vi "Process.vi"(8 "error in":errorcluster, 11 "Lockin.UI":refnum<class "Instrument UI.Lockin.lvclass">) -> (0 "error out":errorcluster, 3 "Lockin.UI out":refnum<class "Instrument UI.Lockin.lvclass">)   [LabVIEW 2019, in "Instrument.Lockin.lvlib" / "Instrument UI.Lockin.lvclass"]
doc: "---------------------------------------------------------------\nJKI State Machine Objects™\nhttp://jki.net/state-machine-objects/\nCopyright (C) 2005-2015, JKI <info@jki.net>\nALL RIGHTS RESERVEDJKI State Machine Objects (SMO) 1.0.0.5\nJKI - JKI\nCopyright (c) 2016, JKI"
uses:
  Instrument UI.Lockin.lvclass
  Instrument.DAQ/Typedefs/DAQ.Calibration--Cluster--Array.ctl
  Instrument.DAQ/Typedefs/DAQ.Calibration--Cluster.ctl
  Instrument.Lockin/Typedefs/Results Type--Enum.ctl
  Instrument.DAQ/Typedefs/Channel.Gain--Cluster--Array.ctl
  Instrument.DAQ/Typedefs/Channel.Gain--Cluster.ctl
  Instrument.DAQ/Typedefs/Sweep.Channel--Cluster--Array.ctl
  Instrument.DAQ/Typedefs/Sweep.Channel--Cluster.ctl
  Instrument.DAQ/Typedefs/Sweep.Pattern--Enum.ctl
  Instrument.DAQ/Typedefs/DAQ.Configuration--Cluster--Array.ctl
  Instrument.DAQ/Typedefs/DAQ.Configuration--Cluster.ctl
  Instrument.DAQ/Typedefs/DAQ.Config.AO.Range--enum.ctl
  Instrument.DAQ/Typedefs/DAQ.TerminalConfiguration--ring.ctl
  Instrument.DAQ/Typedefs/DAQ.Config.AI.Range--enum.ctl
  Instrument.DAQ/Typedefs/DAQ.Config.AI.Coupling--enum.ctl
  Instrument.DAQ/Typedefs/DAQ.Sampling.Fs Mode--enum.ctl
  Instrument.DAQ/Typedefs/Simulation Mode--enum.ctl
  Instrument.DAQ/Typedefs/AI.Channel--Cluster--Array.ctl
  Instrument.DAQ/Typedefs/AI.Channel--Cluster.ctl
  Instrument.DAQ/Typedefs/AO.Channel--Cluster--Array.ctl
  Instrument.DAQ/Typedefs/AO.Channel--Cluster.ctl
  Instrument.DAQ/Typedefs/AO.Channel.Function--Enum.ctl
  Instrument.DAQ/Typedefs/REF.Channel--Cluster--Array.ctl
  Instrument.DAQ/Typedefs/REF.Channel--Cluster.ctl
  Typedefs/Display-Enum.ctl
  C:/Program Files/National Instruments/LabVIEW 2019/vi.lib/JKI/JKI SMO/SMO/SMO.lvclass
  C:/Program Files/National Instruments/LabVIEW 2019/user.lib/LevyLab/Instrument Framework/Instrument UI/Instrument UI.lvclass
  C:/Program Files/National Instruments/LabVIEW 2019/vi.lib/JKI/JKI SMO/SMO.UI/SMO.UI.lvclass
  Instrument.DAQ/Typedefs/DAQ.Sampling.Sample Mode--Ring.ctl
  Instrument.DAQ/Typedefs/State--enum.ctl
  Instrument.Lockin/Typedefs/API/Lockin.setSweep_Table--cluster.ctl
  Instrument.Lockin/Typedefs/Offset Mode--Enum.ctl
  Instrument.DAQ/Typedefs/PrivateEvents--DAQ.setCalibration.ctl
  Instrument.DAQ/Typedefs/Status--enum.ctl
  <userlib>/LevyLab/Instrument Framework/Instrument UI/Instrument UI.lvclass/Instrument UI.ctl
  Instrument.Lockin/Instrument.Lockin.lvclass
  C:/Program Files/National Instruments/LabVIEW 2019/user.lib/LevyLab/Instrument Framework/Instrument/Instrument.lvclass
  Typedefs/UI.Configuration--Cluster.ctl
  Instrument.DAQ/Typedefs/Configuration.Channels--Cluster.ctl
  Instrument.DAQ/Typedefs/DAQ.Sampling--Cluster.ctl
  Instrument.DAQ/Typedefs/DAQ.Sampling.Sampling--Cluster.ctl
  Instrument.DAQ/Typedefs/Configuration.Prefilter--Cluster.ctl
  Instrument.DAQ/Typedefs/Channel.GainsAndOffsets--Cluster.ctl
  Instrument.DAQ/Typedefs/Configuration.AmplitudeLimit--Cluster.ctl
  Instrument.DAQ/Typedefs/Configuration.DCLimit--Cluster.ctl
  Instrument.DAQ/Typedefs/Configuration.LinkFrequencies--Cluster.ctl
  Instrument.DAQ/Typedefs/Sweep.Configuration--Cluster.ctl
  Instrument.DAQ/Typedefs/Configuration.DutyCycle--Cluster.ctl
  Instrument.Lockin/Typedefs/Lockin.getAllData--Cluster.ctl
  Instrument.DAQ/Typedefs/PublicEvents--DAQ.getWaveforms.ctl
  Instrument.DAQ/Typedefs/Results--Cluster.ctl
  Instrument.DAQ/Typedefs/PublicEvents--DAQ.getSweepWaveforms.ctl
  <userlib>/LevyLab/Configuration/Configuration.lvclass
  Typedefs/UI.References--Cluster.ctl
  Typedefs/UI.References.Booleans--Cluster.ctl
  Typedefs/UI.References.Clusters--Cluster.ctl
  Typedefs/UI.References.Graphs--Cluster.ctl
  <userlib>/LevyLab/Configuration/Configuration.lvclass/Configuration.ctl
  <vilib>/JKI/JKI SMO/SMO/SMO.lvclass/SMO.ctl
  <vilib>/JKI/JKI SMO/SMO.UI/SMO.UI.lvclass/SMO.UI.ctl
  Instrument.Lockin/Typedefs/API/Lockin.setState--cluster.ctl
  Instrument.Lockin/Typedefs/API/Lockin.Commands--Enum.ctl
  Instrument.Lockin/Typedefs/API/Lockin.Commands.Local--Enum.ctl
  Instrument.DAQ/Typedefs/PrivateEvents--DAQ.showUI.ctl
  Instrument.Lockin/Typedefs/API/Lockin.setLogMode--cluster.ctl
  Instrument.Lockin/Typedefs/API/Lockin.setSamplingMode--cluster.ctl
  Instrument.Lockin/Typedefs/API/Lockin.setSamplingFsMode--cluster.ctl
  ea889f97-4432-4e18-8daa-f8276c71e6b3.vi
  e313e854-8cc0-44b2-b8a5-b0d9dd449797.vi
  f60e4b8a-05f4-439c-aeb3-da82266228cf.vi
  5a499ed1-b987-4b60-a17a-49cbc4aa87e6.vi
  11ce9ad4-6d29-4ca4-b8bb-b11228104e6f.vi
  a8738246-2ac0-499e-83b1-af72f8904bf5.vi
  <vilib>/JKI/JKI SMO/SMO/Private/ReftoDVR--SMO.vi
  <vilib>/JKI/JKI SMO/SMO.UI/SMO.UI.ReftoDVR.vi
  11ce9ad4-6d29-4ca4-b8bb-b11228104e6f.vi/189031a7-82a1-4f0a-9ed5-d68f3439fd4c.vi
  11ce9ad4-6d29-4ca4-b8bb-b11228104e6f.vi/de7eedf1-e1e8-4423-8aaa-e1093bc59ae0.vi
  <vilib>/Platform/browser.llb/Open URL in Default Browser (string).vi
  private/Set Plot Visibility (WDTWFGraph).vi
  <vilib>/measure/matone.llb/Extract Single Tone Information 1 Chan.vi
  private/Set Plot Color (WFChart2D).vi
  private/Set Legend (WDTWFGraph).vi
  <vilib>/Waveform/WDTOps.llb/WDT Waveform Duration DBL.vi
  <vilib>/Utility/Data Type/Get Type Information.vi
  <vilib>/Utility/Data Type/Get Numeric Information.vi
  <userlib>/_OpenG.lib/lvdata/lvdata.llb/Unwrap VVariant__ogtk.vi
  <vilib>/JDP Science/JSONtext/Variant to JSON Text.vi
  <userlib>/LevyLab/Instrument Framework/Instrument/API/Instrument.sendMessageToProcess (string).vi
  <userlib>/LevyLab/Instrument Framework/Instrument/Instrument.lvclass
  <vilib>/JDP Science/JSONtext/LVClass Serializer/JSONtext LVClass Serializer.lvclass
  <userlib>/LevyLab/Instrument Framework/Instrument UI/Instrument UI.lvclass
  Instrument.DAQ/Instrument.DAQ.lvclass
  <vilib>/measure/NI_MAPro.lvlib
  <vilib>/JKI/JKI SMO/SMO/SMO.lvclass
  <vilib>/JKI/JKI SMO/SMO.UI/SMO.UI.lvclass
  Lockin.Utilities/Lockin.Utilities.lvlib
  C:/Program Files/National Instruments/LabVIEW 2019/user.lib/LevyLab/Instrument Framework/Instrument Types/Lockin/Instrument.LockinAPI.lvclass
  private/Set All Plot Visibility (WFGraph).vi
  private/Set All Plot Visibility (XYGraph).vi
  private/Get Plot Visibility (WFGraph).vi
  private/Set Plot Visibility (WFGraph).vi
  private/Set Plot Visibility (XYGraph).vi
  private/Set Legend (WFGraph).vi
  private/Set Plot Color (WDTWFGraph).vi
  private/Set Plot Color (WFGraph).vi
  private/Set Legend (XYGraph).vi
  private/Set Plot Color (XYGraph).vi
  <vilib>/measure/maspectr.llb/FFT Power Spectrum and PSD for N Chan.vi
panel:
  out "Version":string="vDevelopment" caption="V"
  in  "Fs Multiplier":dbl=5000.0 format="%#_13g"
  in  "Refresh Rate (Hz)":dbl=10.0 format="%#_13g"
  in  "Decimate":enum16{"1", "10", "100", "1000"}(ring) caption="Enum 3"
  in  "Decimation (pre DSP)":i32=1
  in  "Decimation (post DSP)":i32=1
  in  "....................State....................":bool
  in  "....................Graph and UI....................":bool
  in  "....................DAQ and Channel....................":bool
  in  "....................Dynamic Events....................":bool
  in  "Left Tab":T1(tab)=enum."DAQ Settings"
  out "-3dB BW (Hz)":dbl=50.0
  out "Noise BW (Hz)":dbl=50.0
  out "Settling Time (s)":dbl=50.0
  in  "REF Channels":T2 {"Roll-Off" min=1 max=4; "TC" min=1e-06 max=100.0 format="%#_3p"; "Phase" format="%#_3p"; "Frequency" min=1e-06 max=102400.0 format="%#_6p"; "Channel" min=1}
  in  "f link (Hz)":dbl=13.0 format="%#_6p"
  in  "Link f?":bool
  in  "Limit DC?":bool
  in  "AO DC Limit":dbl=0.009999999 caption="DC limit" format="%#_6p"
  in  "Limit AC?":bool
  in  "AC Limit":dbl=0.009999999 caption="AC limit" format="%#_6p"
  in  "duty cycle (%)":dbl=50.0
  in  "Disable All":bool
  in  "Enable All":bool
  in  "AI Channels":T4 {"reference index" min=1; "References" items=["", "1", "2", "3", "4", "5", "6", "7", "8", "9"]; "Channel" min=1}
  in  "AO Channels":T6 {"Phase" format="%#_3g"; "Frequency" min=0.0001 max=200000.0 format="%#_6p"; "Offset" format="%#_6p"; "Amplitude" min=0.0 max=10.0 format="%#_6p"}
  in  "Measure Offset":bool caption="Measure"
  in  "Remove Offset":bool caption="Remove"
  out "Fs Output (S/s)":dbl=100.0
  in  "Fs (S/s) (buffer)":dbl=204800.0 format="%#_13g"
  in  "#s (S) (buffer)":i32=20480
  in  "Show DAQ UI":bool
  out "Fs (S/s)":dbl=10.0 format="%#_13g"
  out "#s (S)":i32=10
  in  "DAQ Config":T9 {"AI terminal config" items=[""=-1, "differential"=10106, "pseudodifferential"=12529]; "AI.Coupling" items=[""=0, "AC"=10045, "DC"=10050, "GND"=10066]; "AO terminal config" items=[""=-1, "differential"=10106, "pseudodifferential"=12529]}
  in  "Auto DAQ":bool caption="Auto Configure"
  in  "Fs Mode":T15
  in  "Logging":bool
  in  "AI Simulation mode":T16=enum."AI = noise*AO"
  in  "Reset Phase":bool
  in  "LP f (Hz)":dbl=100.0 format="%.3p"
  in  "Line":bool
  in  "Lowpass":bool
  in  "PLL AI Channel":i32=1 caption="AI Channel"
  in  "Enable PLL":bool caption="Enable"
  in  "Input Gain":T17
  in  "Output Gain":T17
  in  "Input Offsets":T17 {"Gain" format="%#_3p"}
  in  "Route Signal Type":T19 caption="Signal Type"
  in  "Route Ref Channel":i32=1 caption="Ref Channel"
  in  "Route AI Channel":i32=1 caption="AI Channel"
  out "Route Output (V)":dbl caption="Output (V)"
  in  "Route AO Channel":i32=1 caption="AO Channel" min=1
  in  "Enable Route":bool caption="Enable"
  in  "Sweep Pattern":cluster{"Channel":u16, "Sweep Pattern":dbl[]}[](array[cluster])=[{"Channel"=0, "Sweep Pattern"=[]}] {"Sweep Pattern" format="%#_3p"; "Channel" min=1 max=128}
  in  "Sweep Channels":T20=[{"Enable?"=FALSE, "Channel"=0, "Start"=0.0, "End"=0.1, "Pattern"=enum."Table", "Table"=[]}] {"Table" format="%#_1f"; "Channel" min=1 max=128; "Start" format="%#_6p"; "End" format="%#_6p"}
  in  "Sweep Time (s)":dbl=20.0
  in  "Initial Wait (s)":dbl=1.0
  out "Sweep Timer (s)":dbl caption="Timer (s)"
  in  "Return to Start?":bool
  out "System Serial Number":string caption="SMO State"
  out "Application Version":string caption="SMO State"
  out "Status":string
  out "Sampling Status":u32(colorbox)
  out "State Queue":string
  out "Sampling Status":string="Good"
  out "State History":string
  out "Wfm Refresh Time (ms)":u32=103
  out "Inst.DAQ State":string caption="SMO State"
  out "UI Refresh Time (ms)":u32=103
  out "Sweep Time":dbl format="%<%I:%M:%S %p %m/%d/%Y>T"
  out "State Time":dbl format="%<%I:%M:%S %p %m/%d/%Y>T"
  out "Cal Info":T23 {"DevTemp" format="%.1f"; "SelfCal.LastTemp" format="%.1f"; "SelfCal.LastDate/Time" format="%<%I:%M %p %m/%d/%Y>T"}
  in  "Get Calibration":bool
  in  "Self Calibrate":bool
  in  "Tab Control 3":enum32{"Page 1"}(tab)
  out "mean (V)":dbl format="%_3p"
  out "X (V)":dbl format="%_3p"
  out "Y (V)":dbl format="%_3p"
  in  "channel-reference":u16(ring) items=["AI1 REF 1"]
  out "R (V)":dbl format="%_3p"
  out "theta (°)":dbl format="%_3p"
  in  "Close":bool
  out "String":string
  in  "Pause":bool
  in  "Reset":bool
  in  "Start":bool
  in  "Help":bool
  in  "Start Sweep":bool
  in  "Stop Sweep":bool
  in  "Right Tab":T25(tab)
  in  "Sync?":bool
  in  "Sync Ch":i32=1
  out "f (Hz)":string
  out "phi (°)":string
  in  "Output":enum16{"AO", "REF"}(ring) caption="Enum 3"
  in  "Input":enum16{"Device", "ADC"}(ring) caption="Enum 3"
  out "REF Graph":waveform(dbl)[](graph)
  in  "AO Graph All":bool
  in  "AO Graph None":bool
  in  "AI Graph All":bool
  in  "AI Graph None":bool
  out "AI Graph":waveform(dbl)[](graph)
  in  "X Scale":enum16{"time", "samples"}(ring) caption="Enum 3"
  out "AO Graph":waveform(dbl)[](graph)
  in  "REF Graph None":bool
  in  "REF Graph All":bool
  out "Lockin 1":waveform(dbl)[](graph)
  in  "Display 2":T26 caption="Enum 3"
  in  "Y/Theta Range":dbl caption="Range" format="%#_6p"
  in  "Display 1":T26 caption="Enum 3"
  in  "X/R Range":dbl caption="Range" format="%#_6p"
  out "Lockin 2":waveform(dbl)[](graph)
  in  "Lockin Graph All":bool
  in  "Lockin Graph None":bool
  out "Results":string[][](table)
  out "Lockin XY":cluster{dbl[], dbl[]}[](graph)
  in  "XY Range":dbl caption="Range" format="%#_6p"
  in  "Lockin Graph None 2":bool
  in  "Lockin Graph All 2":bool
  out "Sweep AI":waveform(dbl)[](graph)
  out "Sweep AO":waveform(dbl)[](graph)
  out "Sweep Y":waveform(dbl)[](graph)
  out "Sweep X":waveform(dbl)[](graph)
  in  "chart?":bool=TRUE
  in  "chart all?":bool=TRUE
  in  "PS Display":enum16{"AO", "AI", "X", "Y", "R", "Theta"}(ring) caption="Enum 3"
  in  "# averages":u32=10 min=1
  in  "weighting mode":enum16{"Linear", "Exponential"}(ring)=enum."Exponential"
  in  "averaging mode":T27(ring)=enum."RMS averaging"
  in  "window":u32(ring)=1 items=["Rectangle"=0, "Hanning"=1, "Hamming"=2, "Blackman-Harris"=3, "Exact Blackman"=4, "Blackman"=5, "Flat Top"=6, "4 Term B-Harris "=7, "7 Term B-Harris"=8, "Low Sidelobe"=9, "Blackman Nuttall"=11, "Triangle"=30, "Bartlett-Hanning"=31, "Bohman"=32, "Parzen"=33, "Welch"=34, "Kaiser"=60, "Dolph-Chebyshev"=61, "Gaussian"=62]
  in  "export mode":u16(ring)=1 items=["Power Spectrum", "Power Spectral Density"]
  in  "restart":bool
  out "done?":bool=TRUE
  out "PS Waveform":cluster{"f0":dbl, "df":dbl, "magnitude":dbl[]}[](graph)
  out "averages":dbl=180.0
  out "PS Chart":dbl[][](graph)
  # "Lockin UI"
  # "For instructions on how to use the JKI State Machine Objects, examples and video tutorials, visit:\nhttp://jki.net/state-machine-objects/\n\nJKI State Machine Objects™\nhttp://jki.net/state-machine-objects/\nCopyright (C) 2005-2015, JKI <info@jki.net>\nALL RIGHTS RESERVED"
  # "- Choose an input lockin channel and value (X,Y, etc) and it will be written as a DC value to an output channel of your choosing.\n- Output is scaled by the input amplifier gain."
  # "Output"
  # "Input"
  # ">> DEVICE >>"
  # "(*)"
  # "ch"
  # "AC (V)"
  # "DC (V)"
  # "f (Hz)"
  # "phase (°)"
  # "function"
  # "sweep"
  # "(*)"
  # "ch"
  # "1     2    3"
  # "References"
  # "Offset"
  # "Output Settings"
  # "Reference"
  # "Reference Filter"
  # "ch"
  # "f (Hz)"
  # "phase (°)"
  # "TC (s)"
  # "order (n)"
  # "DAQ Channels"
  # "Device"
  # "AO"
  # "AI"
  # "terminals"
  # "ch"
  # "ch"
  # "range"
  # "range"
  # "coupling"
  # "terminals"
  # "Sampling"
  # "Pre-Filters"
  # "Simulation"
  # "Push \"Reset Acquisiton\" below when you want to apply new settings"
  # "not used during process-ing"
  # "DAQ"
  # "Logging"
  # "Output Gain"
  # "Input Offset / Gain"
  # "Route Lockin Input to Output"
  # "PLL"
  # "experimental ca 11/18/2025"
  # "experimental ca 11/18/2025"
  # "ch"
  # "Input gain"
  # "ch"
  # "Output gain"
  # "ch"
  # "Input offset"
  # "Sweep"
  # "pattern"
  # "(*)"
  # "ch"
  # "start"
  # "end"
  # "ch"
  # "table"
  # "Status"
  # "Calibration"
  # "Most Recent Self-Calibration"
  # "device"
  # "time"
  # "T (°C)"
  # "T (°C)"
  # "OK?"
  # "DAQ"
  # "Sweep"
  # "Application"
  # "Status"
  # "Input Graphs"
  # "Output Graphs"
  # "Lockin Results: Graph 1"
  # "Lockin Results: Graph 2"
  # "Lockin Results: Table"
  # "Lockin Results: Phasor Graph"
  # "Sweep AI"
  # "Sweep AO"
  # "Sweep Results"
  # "Sweep Results"
  # "Power Spectra"
  # "db( ):\ndB(V) for volts\ndB(A) for amps\ndB(°) for degrees"
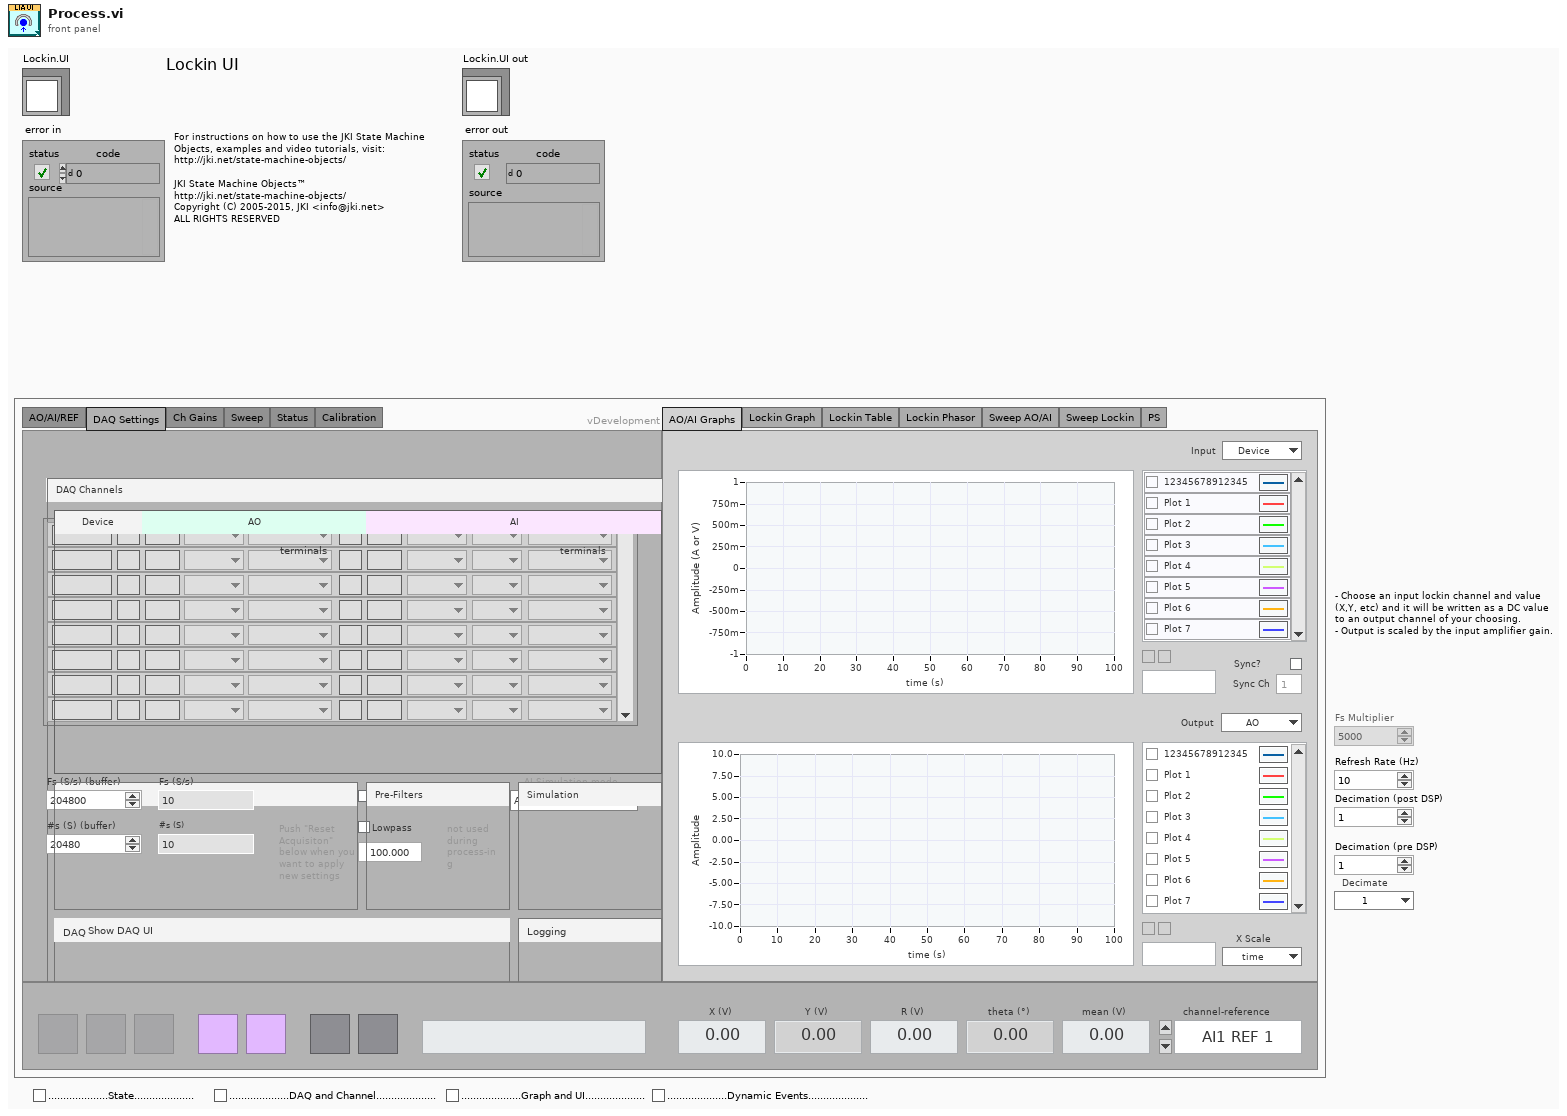
[diagram p1: front panel]
types:
  T1 = enum32{"AO/AI/REF", "DAQ Settings", "Ch Gains", "Sweep", "Status", "Calibration"}
  T2 = typedef "Instrument.Lockin.lvlib/Instrument.DAQ.lvclass/REF.Channel--Cluster--Array.ctl" = T3[]
  T3 = typedef "Instrument.Lockin.lvlib/Instrument.DAQ.lvclass/REF.Channel--Cluster.ctl" = cluster{"Enable?":bool, "Channel":i32, "Frequency":dbl, "Phase":dbl, "TC":dbl, "Roll-Off":i32}
  T4 = typedef "Instrument.Lockin.lvlib/Instrument.DAQ.lvclass/AI.Channel--Cluster--Array.ctl" = T5[]
  T5 = typedef "Instrument.Lockin.lvlib/Instrument.DAQ.lvclass/AI.Channel--Cluster.ctl" = cluster{"Enable?":bool, "Channel":i32, "References":u16[], "reference index":i32}
  T6 = typedef "Instrument.Lockin.lvlib/Instrument.DAQ.lvclass/AO.Channel--Cluster--Array.ctl" = T7[]
  T7 = typedef "Instrument.Lockin.lvlib/Instrument.DAQ.lvclass/AO.Channel--Cluster.ctl" = cluster{"Enable?":bool, "Channel":i32, "Amplitude":dbl, "Offset":dbl, "Frequency":dbl, "Phase":dbl, "Function":T8, "Sweeping?":bool, "Limit AC":bool, "Limit DC?":bool, "Duty Cycle":bool}
  T8 = typedef "Instrument.Lockin.lvlib/Instrument.DAQ.lvclass/AO.Channel.Function--Enum.ctl" = enum16{"sine", "square", "triangle", "saw"}
  T9 = typedef "Instrument.Lockin.lvlib/Instrument.DAQ.lvclass/DAQ.Configuration--Cluster--Array.ctl" = T10[]
  T10 = typedef "Instrument.Lockin.lvlib/Instrument.DAQ.lvclass/DAQ.Configuration--Cluster.ctl" = cluster{"Device":string, "Lockin.AO":string, "AO.Ch":string, "AO.Range":T11, "AO terminal config":T12, "Lockin.AI":string, "AI.Ch":string, "AI.Range":T13, "AI.Coupling":T14, "AI terminal config":T12}
  T11 = typedef "Instrument.Lockin.lvlib/Instrument.DAQ.lvclass/DAQ.Config.AO.Range--enum.ctl" = enum16{"±0.1", "±1.0", "±3.5", "±10.0", ""}
  T12 = typedef "Instrument.Lockin.lvlib/Instrument.DAQ.lvclass/DAQ.TerminalConfiguration--ring.ctl" = i32
  T13 = typedef "Instrument.Lockin.lvlib/Instrument.DAQ.lvclass/DAQ.Config.AI.Range--enum.ctl" = enum16{"±0.316", "±1.00", "±3.16", "±10.0", "±31.6", "±42.4", ""}
  T14 = typedef "Instrument.Lockin.lvlib/Instrument.DAQ.lvclass/DAQ.Config.AI.Coupling--enum.ctl" = u16
  T15 = typedef "Instrument.Lockin.lvlib/Instrument.DAQ.lvclass/DAQ.Sampling.Fs Mode--enum.ctl" = enum16{"Manual", "Auto Fs", "Max Fs"}
  T16 = typedef "Instrument.Lockin.lvlib/Instrument.DAQ.lvclass/Simulation Mode--enum.ctl" = enum16{"AI = HW simulated", "AI = noise*AO", "AI = waveguide"}
  T17 = typedef "Instrument.Lockin.lvlib/Instrument.DAQ.lvclass/Channel.Gain--Cluster--Array.ctl" = T18[]
  T18 = typedef "Instrument.Lockin.lvlib/Instrument.DAQ.lvclass/Channel.Gain--Cluster.ctl" = cluster{"Channel":string, "Gain":dbl}
  T19 = typedef "Instrument.Lockin.lvlib/Instrument.Lockin.lvclass/Results Type--Enum.ctl" = enum16{"X", "Y", "R", "Theta", "Mean"}
  T20 = typedef "Instrument.Lockin.lvlib/Instrument.DAQ.lvclass/Sweep.Channel--Cluster--Array.ctl" = T21[]
  T21 = typedef "Instrument.Lockin.lvlib/Instrument.DAQ.lvclass/Sweep.Channel--Cluster.ctl" = cluster{"Enable?":bool, "Channel":u16, "Start":dbl, "End":dbl, "Pattern":T22, "Table":dbl[]}
  T22 = typedef "Instrument.Lockin.lvlib/Instrument.DAQ.lvclass/Sweep.Pattern--Enum.ctl" = enum16{"Ramp /", "Ramp /\\", "Smooth Ramp _/", "Smooth Ramp _/\\_", "Table"}
  T23 = typedef "Instrument.Lockin.lvlib/Instrument.DAQ.lvclass/DAQ.Calibration--Cluster--Array.ctl" = T24[]
  T24 = typedef "Instrument.Lockin.lvlib/Instrument.DAQ.lvclass/DAQ.Calibration--Cluster.ctl" = cluster{"Active Device":string, "SelfCal.LastDate/Time":dbl, "SelfCal.LastTemp":dbl, "DevTemp":dbl, "calibration due?":bool}
  T25 = enum32{"AO/AI Graphs", "Lockin Graph", "Lockin Table", "Lockin Phasor", "Sweep AO/AI", "Sweep Lockin", "PS"}
  T26 = typedef "Instrument.Lockin.lvlib/Instrument UI.Lockin.lvclass/Display-Enum.ctl" = enum16{"X", "Y", "R", "Theta", "Mean"}
  T27 = enum16{"No averaging", "Vector averaging", "RMS averaging", "Peak hold"}
  T28 = enum16{"Spinner 1", "Spinner 2", "Spinner 3", "Spinner 4", "Spinner 5", "Spinner 6"}
  T29 = typedef "Instrument.Lockin.lvlib/Instrument.DAQ.lvclass/State--enum.ctl" = enum16{"start", "stop", "reset", "start sweep", "stop sweep"}
  T30 = typedef "Instrument.Lockin.lvlib/Instrument.Lockin.lvclass/Lockin.setSweep_Table--cluster.ctl" = cluster{"Channel":i32, "Table":dbl[]}
  T31 = typedef "Instrument.Lockin.lvlib/Instrument.Lockin.lvclass/Offset Mode--Enum.ctl" = enum16{"Measure", "Remove"}
  T32 = typedef "Instrument.Lockin.lvlib/Instrument.DAQ.lvclass/PrivateEvents--DAQ.setCalibration.ctl" = enum16{"Check", "Calibrate"}
  T33 = typedef "Instrument.Lockin.lvlib/Instrument.DAQ.lvclass/Status--enum.ctl" = enum16{"idle", "created", "started", "stopped", "sweeping"}
  T34 = enum32{"invalid app kind", "Development System", "Run Time System", "Student Edition", "Embedded LabVIEW", "Evaluation", "Custom"}
  T35 = enum32{"Invalid", "Standard", "Closed", "Hidden", "Minimized", "Maximized"}
  T36 = enum8{"Enabled", "Disabled", "Disabled and Grayed Out"}
  T37 = typedef "Instrument.Lockin.lvlib/Instrument.Lockin.lvclass/Lockin.setState--cluster.ctl" = cluster{"State":T29}
  T38 = typedef "Instrument.Lockin.lvlib/Instrument.Lockin.lvclass/Lockin.Commands--Enum.ctl" = enum16{"setAO", "setAO_Amplitude", "setAO_DC", "setAO_Frequency", "setAO_Phase", "setAO_Function", "setREF", "setREF_Frequency", "setREF_Phase", "setREF_TC", "setREF_Roll-Off", "setDAQ", "setSampling", "setState", "getState", "getAO", "getAI", "getResults", "getSampling", "getAOconfig", "getREFconfig", "setInputGain", "setOutputGain", "getInputGain", "getOutputGain", "setSamplingFsMode", "getSamplingFsMode", "setSweep", "setSweep_Time", "setSweep_Table", "getStatus", "getSweepResults", "getSweepWaveforms", "logConfiguration", "startLogging", "stopLogging"}
  T39 = typedef "Instrument.Lockin.lvlib/Instrument.Lockin.lvclass/Lockin.Commands.Local--Enum.ctl" = enum16{"autoConfigureDAQ", "setSimulationMode", "zeroPhase", "setCalibration", "setPreFilter", "setFrequencyLink", "setAmplitudeLimit", "setDCLimit", "setDutyCycle", "setSamplingDecimationPreDSP", "setSamplingDecimationPostDSP", "setSamplingMode", "setSamplingFsMultiplier", "setSamplingFsOutput", "setSamplingRefreshRate", "setData_State", "setData_DAQ", "setData_Sampling", "setData_Waveforms", "setData_Results", "setData_SweepWaveforms", "setData_AIChannels", "setData_AOChannels", "setData_REFChannels", "setData_InputGain", "setData_OutputGain", "showUI", "setAI", "setOffset", "setOffsetMode"}
  T40 = typedef "Instrument.Lockin.lvlib/Instrument.DAQ.lvclass/PrivateEvents--DAQ.showUI.ctl" = bool
  T41 = typedef "Instrument.Lockin.lvlib/Instrument.Lockin.lvclass/Lockin.setLogMode--cluster.ctl" = cluster{"interval":u32}
  T42 = typedef "Instrument.Lockin.lvlib/Instrument.Lockin.lvclass/Lockin.setSamplingMode--cluster.ctl" = cluster{"SampleMode":T43}
  T43 = typedef "Instrument.Lockin.lvlib/Instrument.DAQ.lvclass/DAQ.Sampling.Sample Mode--Ring.ctl" = i32
  T44 = typedef "Instrument.Lockin.lvlib/Instrument.Lockin.lvclass/Lockin.setSamplingFsMode--cluster.ctl" = cluster{"FsMode":T15}
  T45 = cluster{"averaging mode":enum16{"No averaging", "Vector averaging", "RMS averaging", "Peak hold"}, "weighting mode":enum16{"Linear", "Exponential"}, "number of averages":u32}
  T46 = typedef "Instrument.Lockin.lvlib/Instrument UI.Lockin.lvclass/UI.Configuration--Cluster.ctl" = cluster{"Channels":T47, "DAQ":cluster{"Configuration":T9, "cfg.Sampling":T48, "Calibration":T23, "Simulation mode":T16}, "PreFilter":T50, "Amplifers":T51, "Limit Amplitude":T52, "Limit DC":T53, "Link Frequencies":T54, "Sweep":T55, "Plot":cluster{"visibility.AI":bool[], "visibility.AO":bool[], "visibility.Lockin":bool[], "Display 1":T26, "Display 2":T26}, "Function Option":T56}
  T47 = typedef "Instrument.Lockin.lvlib/Instrument.DAQ.lvclass/Configuration.Channels--Cluster.ctl" = cluster{"Cfg_AO":T6, "Cfg_AI":T4, "Cfg_REF":T2}
  T48 = typedef "Instrument.Lockin.lvlib/Instrument.DAQ.lvclass/DAQ.Sampling--Cluster.ctl" = cluster{"Sampling":T49, "sample mode":i32, "Fs Mode":T15, "Fs Multiplier":dbl, "Refresh Rate (Hz)":dbl, "Decimation.PreDSP":i32, "Decimation.PostDSP":i32, "Fs.Output":dbl}
  T49 = typedef "Instrument.Lockin.lvlib/Instrument.DAQ.lvclass/DAQ.Sampling.Sampling--Cluster.ctl" = cluster{"Fs":dbl, "#s":i32}
  T50 = typedef "Instrument.Lockin.lvlib/Instrument.DAQ.lvclass/Configuration.Prefilter--Cluster.ctl" = cluster{"60 Hz":bool, "Low Pass":bool, "Low Pass Cutoff (Hz)":dbl}
  T51 = typedef "Instrument.Lockin.lvlib/Instrument.DAQ.lvclass/Channel.GainsAndOffsets--Cluster.ctl" = cluster{"Offset_AI":T17, "Gain_AI":T17, "Gain_AO":T17}
  T52 = typedef "Instrument.Lockin.lvlib/Instrument.DAQ.lvclass/Configuration.AmplitudeLimit--Cluster.ctl" = cluster{"Limit?":bool, "Limit (V)":dbl}
  T53 = typedef "Instrument.Lockin.lvlib/Instrument.DAQ.lvclass/Configuration.DCLimit--Cluster.ctl" = cluster{"Limit?":bool, "Limit (V)":dbl}
  T54 = typedef "Instrument.Lockin.lvlib/Instrument.DAQ.lvclass/Configuration.LinkFrequencies--Cluster.ctl" = cluster{"Link?":bool, "Frequency (Hz)":dbl}
  T55 = typedef "Instrument.Lockin.lvlib/Instrument.DAQ.lvclass/Sweep.Configuration--Cluster.ctl" = cluster{"sweepTime":dbl, "initialWaitTime":dbl, "returnToStart":bool, "sweepChannels":T20}
  T56 = typedef "Instrument.Lockin.lvlib/Instrument.DAQ.lvclass/Configuration.DutyCycle--Cluster.ctl" = cluster{"Option?":bool, "Duty Cycle (%)":dbl}
  T57 = typedef "Instrument.Lockin.lvlib/Instrument.Lockin.lvclass/Lockin.getAllData--Cluster.ctl" = cluster{"DAQ State":T33, "Waveforms":T58, "Results":T59, "SweepWaveforms":T60}
  T58 = typedef "Instrument.Lockin.lvlib/Instrument.DAQ.lvclass/PublicEvents--DAQ.getWaveforms.ctl" = cluster{"AO":waveform(dbl)[], "AI":waveform(dbl)[], "REF_X":waveform(dbl)[], "REF_Y":waveform(dbl)[], "X":waveform(dbl)[], "Y":waveform(dbl)[]}
  T59 = typedef "Instrument.Lockin.lvlib/Instrument.DAQ.lvclass/Results--Cluster.ctl" = cluster{"Time Stamp":timestamp, "Results (Dictionary)":cluster{"key":string, "value":dbl[]}[]}
  T60 = typedef "Instrument.Lockin.lvlib/Instrument.DAQ.lvclass/PublicEvents--DAQ.getSweepWaveforms.ctl" = cluster{"AO":waveform(dbl)[], "AI":waveform(dbl)[], "X":waveform(dbl)[], "Y":waveform(dbl)[]}
  T61 = typedef "Instrument.Lockin.lvlib/Instrument UI.Lockin.lvclass/UI.References--Cluster.ctl" = cluster{"Booleans":T62, "Clusters":T63, "Graphs":T64}
  T62 = typedef "Instrument.Lockin.lvlib/Instrument UI.Lockin.lvclass/UI.References.Booleans--Cluster.ctl" = cluster{"Start":refnum<vi>, "Pause":refnum<vi>, "Reset":refnum<vi>, "Trigger":refnum<vi>, "Help":refnum<vi>, "Close":refnum<vi>, "Start Sweep":refnum<vi>, "Stop Sweep":refnum<vi>}
  T63 = typedef "Instrument.Lockin.lvlib/Instrument UI.Lockin.lvclass/UI.References.Clusters--Cluster.ctl" = cluster{"AO Channels":refnum<vi>, "AI Channels":refnum<vi>, "REF Channels":refnum<vi>, "DAQ Config":refnum<vi>, "Sweep Channels":refnum<vi>, "Cal Info":refnum<vi>}
  T64 = typedef "Instrument.Lockin.lvlib/Instrument UI.Lockin.lvclass/UI.References.Graphs--Cluster.ctl" = cluster{"AI Graph":refnum<vi>, "AO Graph":refnum<vi>, "REF Graph":refnum<vi>, "Lockin 1":refnum<vi>, "Lockin 2":refnum<vi>, "Lockin XY":refnum<vi>, "Sweep X Graph":refnum<vi>, "Sweep Y Graph":refnum<vi>, "Sweep AI Graph":refnum<vi>, "Sweep AO Graph":refnum<vi>, "PS WFGraph":refnum<vi>, "PS Chart":refnum<vi>}
  T65 = cluster{"Core":cluster{"Current VI Reference":refnum<vi>, "Close Panel on Exit?":bool, "Last Error":cluster{"error":errorcluster, "previous state":string, "remaining states":string}, "Shutdown?":bool}, "SelfRef":refnum<class "Instrument UI.Lockin.lvclass">, "Lockin":refnum<class "Instrument.Lockin.lvclass">, "Configuration":refnum<class "Configuration.lvclass">, "UI Config":T46, "DAQ state":T33, "getAll":T57, "Waveform Charts":waveform(dbl)[][], "References":T61, "Message":cluster{"Command":variant, "Data":variant}, "Front Panel":refnum<vi>, "update waveform graphs":bool, "update lockin graphs":bool, "clear lockin charts":bool}
  T66 = cluster{"Enable?":bool, "Channel":bool, "References":bool[], "reference index":bool}[]
  T67 = typedef "SMO.lvclass/SMOState --Enum.ctl" = enum16{"unknown", "Created", "Started", "Stopped"}
  T68 = cluster{"Current VI Reference":refnum<vi>, "Close Panel on Exit?":bool, "Last Error":cluster{"error":errorcluster, "previous state":string, "remaining states":string}, "Shutdown?":bool}
  T69 = typedef "SMO.lvclass/Protected Events.ctl" = cluster{"StopProcesses":refnum<user-event>, "AbortProcesses":refnum<user-event>, "Config Changed":refnum<user-event>, "Dependency":refnum<user-event>}
  T70 = typedef "Instrument.lvlib/Instrument.lvclass/PublicEvents--Cluster.ctl" = cluster{"MessageFromProcess":refnum<user-event>}
  T71 = typedef "SMO.UI.lvclass/PublicEvents--Cluster.ctl" = cluster{"UI Hidden":refnum<user-event>, "UI State":refnum<user-event>}
  T72 = typedef "SMO.lvclass/Public Events.ctl" = cluster{"Error":refnum<user-event>, "State":refnum<user-event>, "Reserve State":refnum<user-event>}
  T73 = typedef "Instrument.Lockin.lvlib/Instrument.DAQ.lvclass/PublicEvents--Cluster.ctl" = cluster{"getAIChannels":refnum<user-event>, "getAOChannels":refnum<user-event>, "getREFChannels":refnum<user-event>, "getWaveforms":refnum<user-event>, "getResults":refnum<user-event>, "getSweepWaveforms":refnum<user-event>, "getCalibration":refnum<user-event>, "getDAQState":refnum<user-event>, "getDAQconfig":refnum<user-event>, "getInputGain":refnum<user-event>, "getOutputGain":refnum<user-event>, "getInputOffset":refnum<user-event>, "getSampling":refnum<user-event>, "getSweepChannels":refnum<user-event>, "getDeviceIDN":refnum<user-event>}
  T74 = typedef "Instrument.lvlib/Instrument.lvclass/Instrument.IDN--cluster.ctl" = cluster{"vendor":string, "model":string, "serial":string, "firmware":string}
  T75 = cluster{"Fs.Output (S/s)":dbl, "Decimation Factor":i32, "Settling Time (s)":dbl, "Noise Bandwidth (Hz)":dbl, "-3dB Bandwidth (Hz)":dbl, "Attenuation (dB)":dbl}
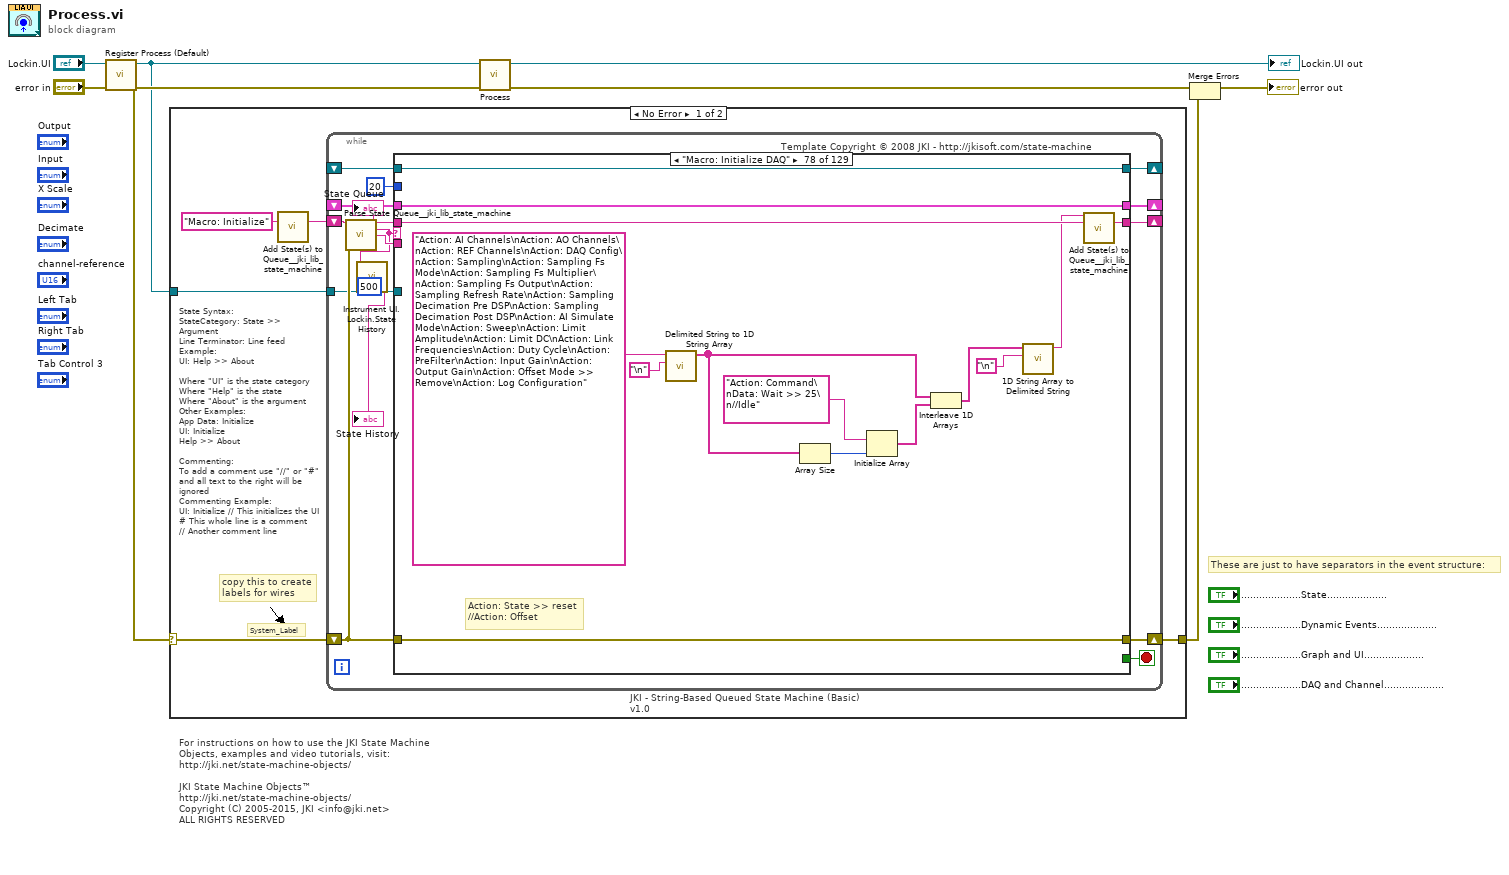
[diagram p0: block diagram]
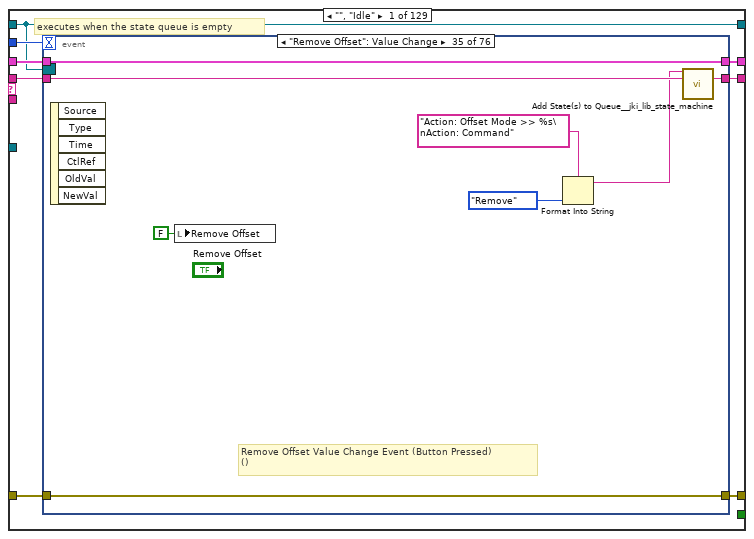
[diagram p2: hidden frame]
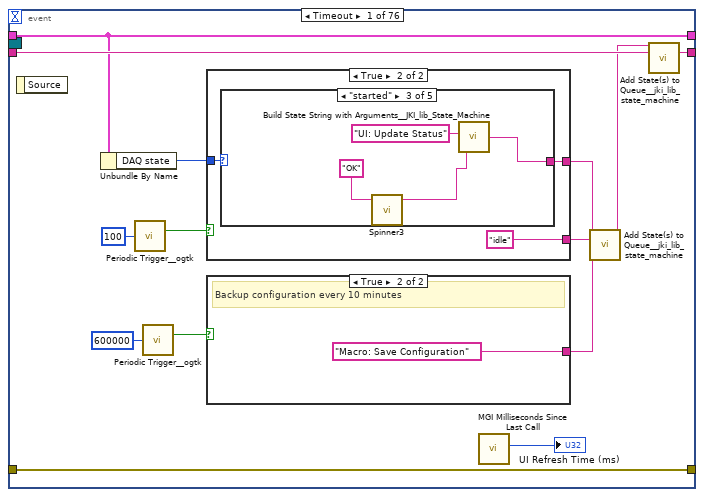
[diagram p3: hidden frame]
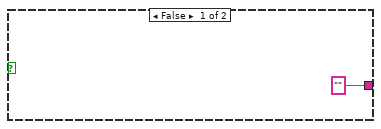
[diagram p4: hidden frame]
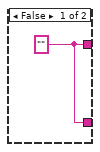
[diagram p5: hidden frame]
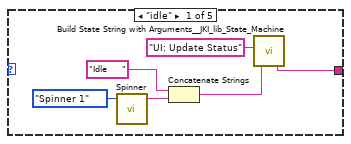
[diagram p6: hidden frame]
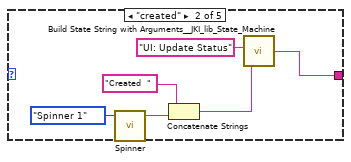
[diagram p7: hidden frame]
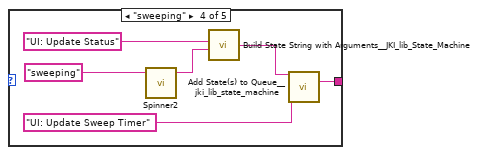
[diagram p8: hidden frame]
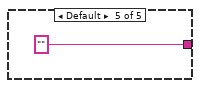
[diagram p9: hidden frame]
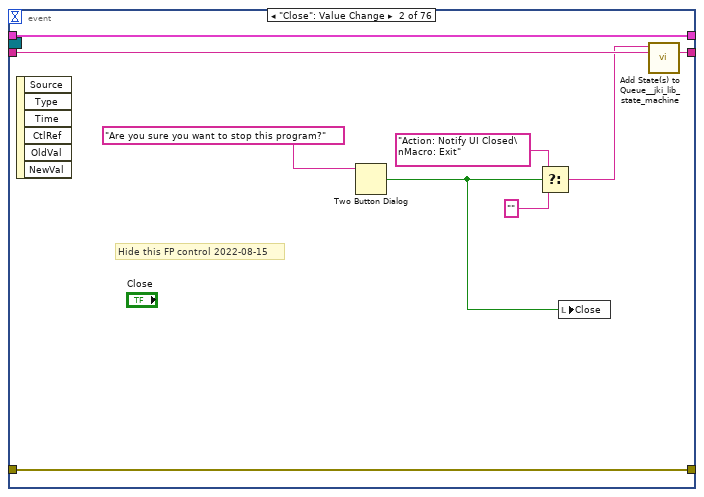
[diagram p10: hidden frame]
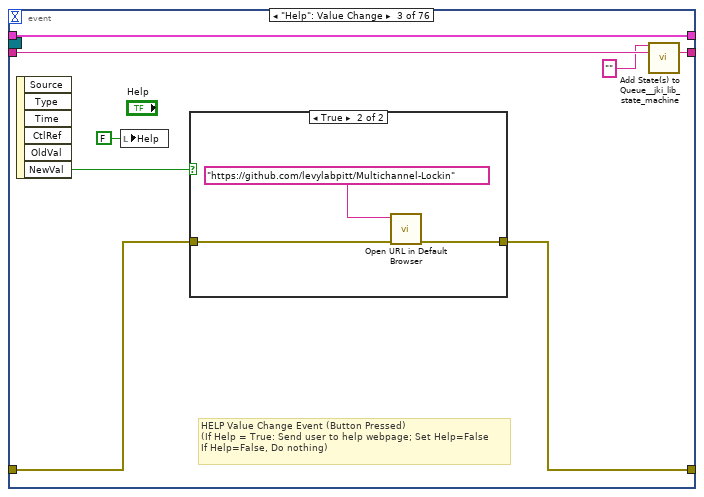
[diagram p11: hidden frame]
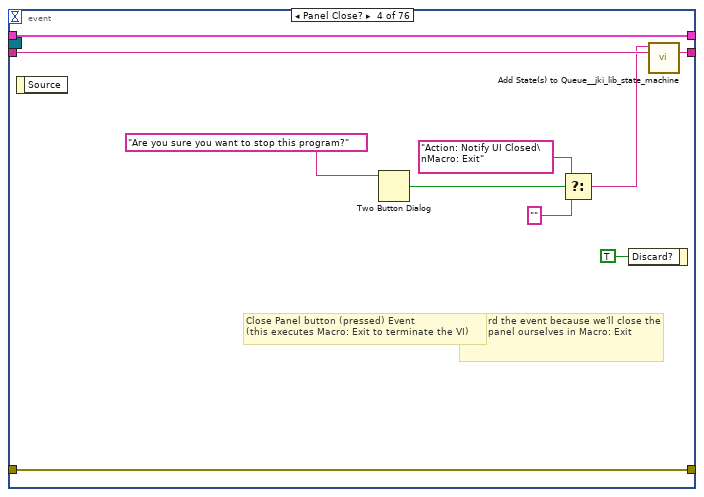
[diagram p13: hidden frame]
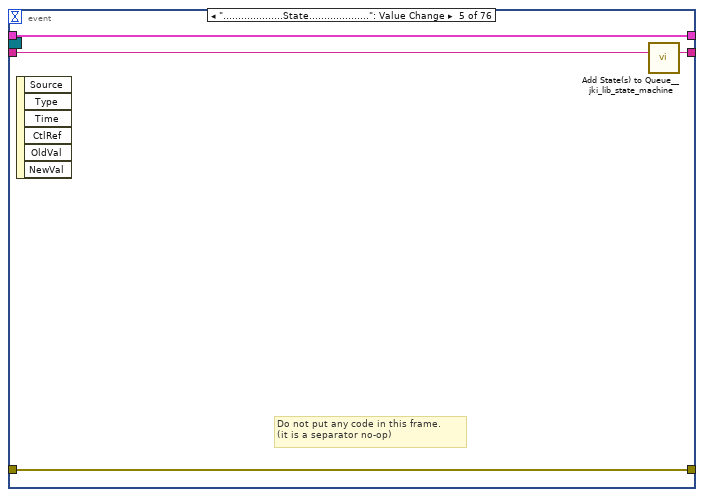
[diagram p14: hidden frame]
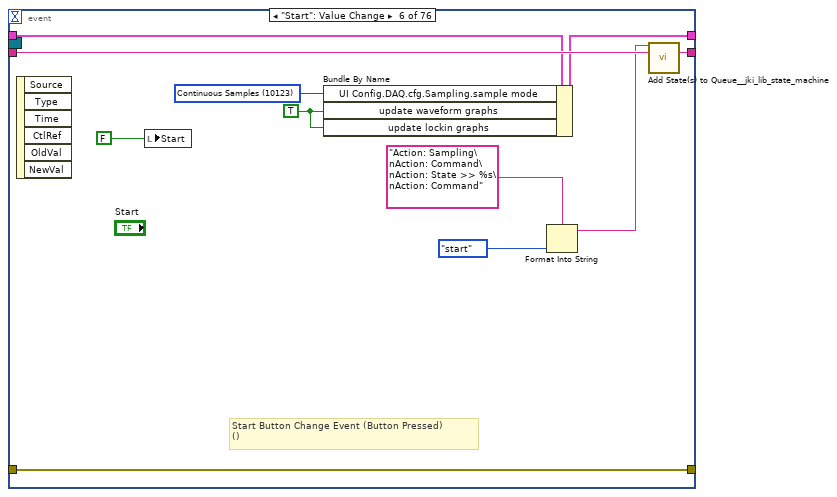
[diagram p15: hidden frame]
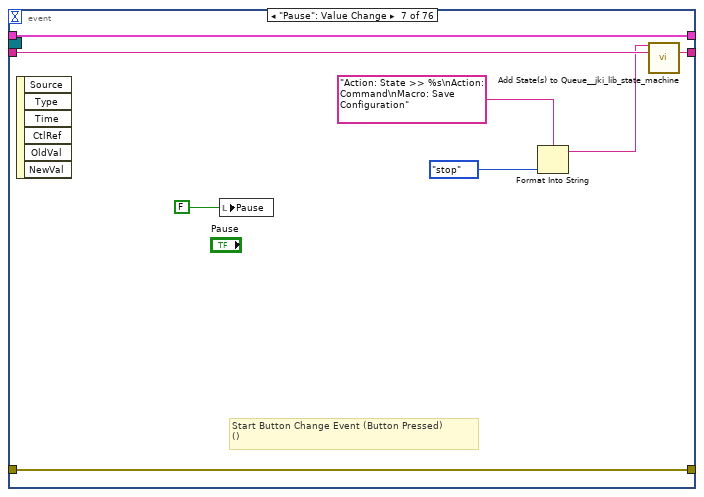
[diagram p16: hidden frame]
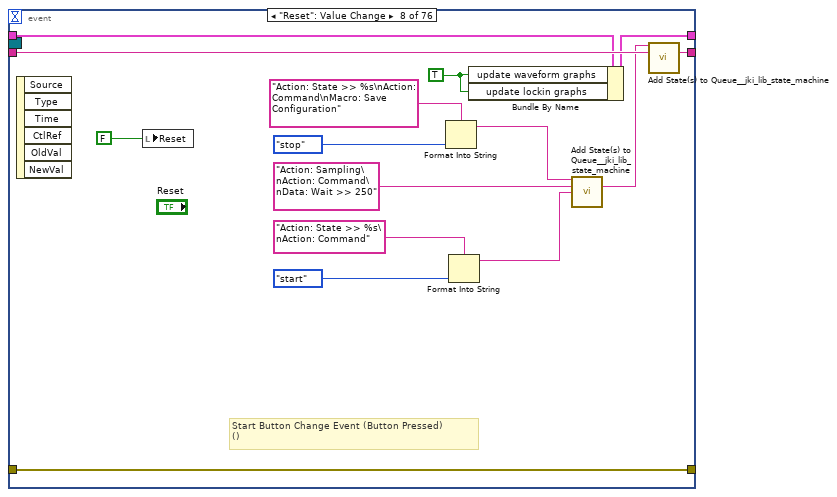
[diagram p17: hidden frame]
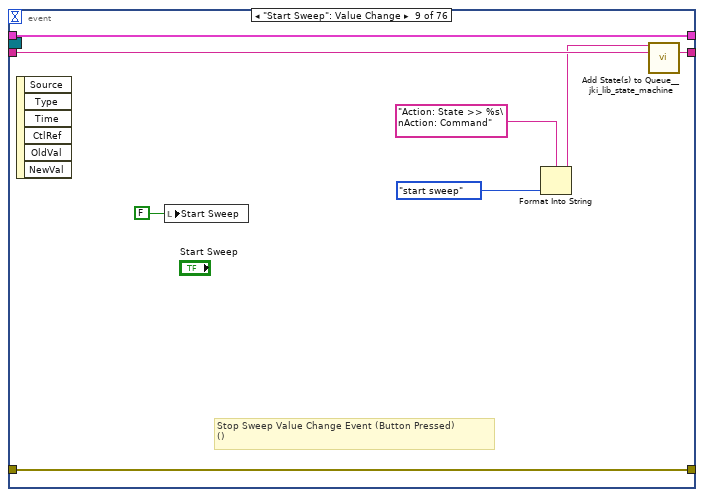
[diagram p18: hidden frame]
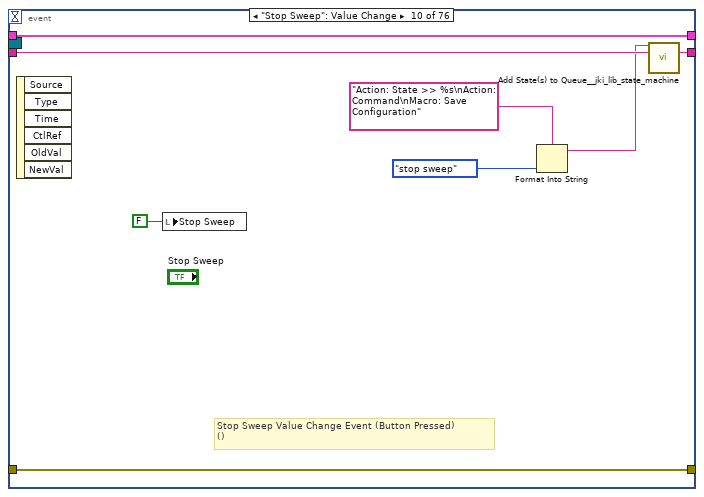
[diagram p19: hidden frame]
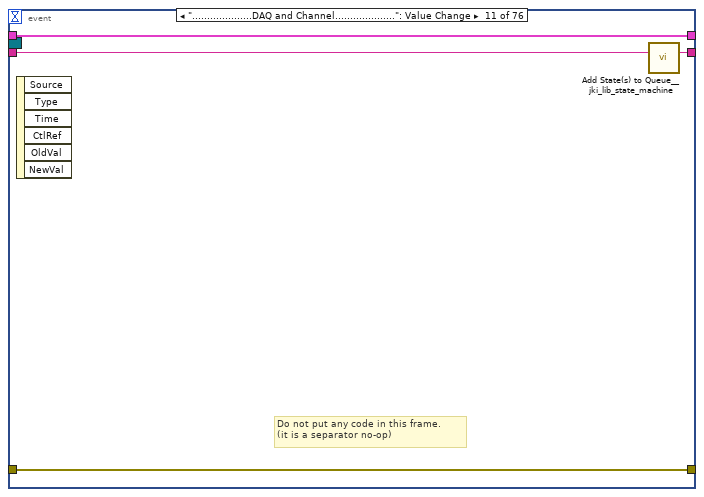
[diagram p20: hidden frame]
diagram:
  # "These are just to have separators in the event structure:"
  # "For instructions on how to use the JKI State Machine Objects, examples and video tutorials, visit:\nhttp://jki.net/state-machine-objects/\n\nJKI State Machine Objects™\nhttp://jki.net/state-machine-objects/\nCopyright (C) 2005-2015, JKI <info@jki.net>\nALL RIGHTS RESERVED"
  n1 = call <vilib>:"Register Process (Default).vi"("error in (no error)"="error in", "SMO"="Lockin.UI") -> ("error out"=w5:errorcluster, "SelfRef"=w4:refnum<class "Instrument UI.Lockin.lvclass">)  [unwired: 8 in]
  n2 = case shown="No Error" w5 {
    selector: w5 -> [w10 w2437]
    tunnel: w4 -> [w11 _]
    tunnel: [w9 w2437] -> w1
    frame No Error {
      # "State Syntax:\nStateCategory: State >> Argument\nLine Terminator: Line feed\nExample:\nUI: Help >> About\n\nWhere \"UI\" is the state category\nWhere \"Help\" is the state\nWhere \"About\" is the argument\nOther Examples:\nApp Data: Initialize\nUI: Initialize\nHelp >> About\n\nCommenting:\nTo add a comment use \"//\" or \"#\" and all text to the right will be ignored\nCommenting Example:\nUI: Initialize // This initializes the UI\n# This whole line is a comment\n// Another comment line"
      # "copy this to create labels for wires"
      # "System_Label"
      n3 = call <vilib>:"Add State(s) to Queue__jki_lib_state_machine.vi"("State(s) in (\"\")"="Macro: Initialize") -> ("States Out"=w13:string)  [unwired: 14 in]
      n4 = while "JKI - String-Based Queued State Machine (Basic) v1.0" {
        shift-right: [w24] -> _
        shift-left: _ -> [w23]
        shift-right: [w27] -> w9
        shift-left: w10 -> [w21]
        shift-right: [w26] -> _
        shift-left: w13 -> [w28]
        tunnel: w11 -> [w20]
        shift-right: [w19] -> _
        shift-left: _ -> [w18]
        stop <- w25 stop-if-true
        # "Template Copyright © 2008 JKI - http://jkisoft.com/state-machine"
        n5 = call <vilib>:"Parse State Queue__jki_lib_state_machine.vi"("State Queue"=w28, "Error In (no error)"=w21) -> ("Remaining States"=w14:string, "Current State"=w17:string, "Arguments"=w29:string)  [unwired: 11 in]
        "State Queue" <- w14
        n6 = call "Instrument UI.Lockin.State History.vi"("history length (100)"=500, "Current State"=w17) -> ("History"=→"State History":string)  [unwired: 9 in]
        n7 = case shown="\"Macro: Initialize DAQ\"" w17 {
          selector: w17 -> [_ _ w730 _ _ _ _ _ _ _ _ _ _ _ _ _ _ _ _ _ _ _ _ _ _ _ _ _ _ _ _ _ _ _ _ _ _ _ _ _ _ _ _ _ _ _ _ _ _ _ _ _ _ _ _ _ _ _ _ _ _ _ _ _ _ _ _ _ _ _ _ _ _ _ _ _ _ _ _ _ _ _ _ _ _ _ _ _ _ _ _ _ _ _ _ _ _ _ _ _ _ _ _ _ _ _ _ _ _ _ _ _ _ _ _ _ _ _ _ _ _ _ _ _ _ _ _ _ _]
          tunnel: w14 -> [w37 w728 w734 w753 w756 w772 w777 w800 w821 w838 w867 w875 w882 w887 w901 w911 w924 w929 w941 w948 w964 w1000 w1008 w1016 w1023 w1029 w1058 w1071 w1100 w1114 w1123 w1131 w1140 w1156 w1189 w1202 w1213 w1232 w1250 w1265 w1278 w1289 w1306 w1341 w1391 w1405 w1418 w1429 w1445 w1452 w1466 w1483 w1508 w1526 w1560 w1584 w1608 w1626 w1637 w1658 w1671 w1691 w1704 w1714 w1726 w1765 w1776 w1791 w1807 w1818 w1848 w1853 w1864 w1876 w1887 w1896 w1905 w1919 w1925 w1931 w1940 w1957 w1963 w1980 w1985 w1996 w2003 w2008 w2027 w2033 w2040 w2045 w2052 w2064 w2076 w2088 w2098 w2116 w2124 w2131 w2139 w2147 w2155 w2165 w2178 w2186 w2197 w2207 w2217 w2225 w2239 w2247 w2255 w2263 w2271 w2279 w2287 w2295 w2303 w2311 w2320 w2331 w2342 w2355 w2365 w2372 w2399 w2429 w2436]
          tunnel: w29 -> [_ _ _ _ _ _ _ _ _ _ _ w868 _ _ _ _ _ _ _ w942 w958 w995 w1003 w1011 _ w1024 _ _ _ _ _ _ _ _ w1181 w1195 w1208 w1226 _ _ _ _ _ _ _ _ _ _ _ _ _ _ _ _ _ _ _ _ _ _ _ _ _ _ _ _ _ w1783 _ w1809 _ _ _ _ _ _ _ _ _ _ _ _ _ _ _ _ _ _ _ _ _ _ _ _ _ w2081 w2092 w2110 _ _ _ _ _ _ _ _ _ _ _ _ _ _ _ _ _ _ _ _ _ _ _ _ _ w2348 w2358 _ _ _ _]
          tunnel: w23 -> [w35 w725 w732 w744 w759 w768 w774 _ w802 w828 w862 w872 w877 w884 w897 w907 w920 w926 w935 w946 w960 w996 w1005 w1013 w1020 w1026 w1039 w1067 w1095 w1103 w1115 w1126 w1136 w1145 w1183 w1197 w1209 w1227 w1247 w1254 w1275 w1286 w1303 w1337 w1388 w1402 w1415 w1426 w1442 w1449 w1463 w1480 w1504 w1521 w1536 w1569 w1605 w1620 w1629 w1654 w1664 w1687 w1701 w1709 w1722 w1762 w1771 w1788 w1804 w1810 w1832 w1850 w1860 w1866 w1884 w1893 w1902 w1916 w1921 w1927 w1932 w1946 w1960 w1966 w1982 w1993 w1998 w2005 w2025 w2031 w2034 w2041 w2048 w2060 w2072 w2083 w2093 w2111 w2119 w2126 w2134 w2142 w2150 w2156 w2173 w2181 w2192 w2202 w2212 w2220 w2234 w2242 w2250 w2258 w2266 w2274 w2282 w2290 w2298 w2306 w2315 w2326 w2335 w2350 w2360 w2367 w2396 w2423 w2430]
          tunnel: [w34 w726 w736 w750 w761 w767 w775 w790 w819 w836 w865 w873 w878 w885 w889 w906 w915 w927 w937 w943 w961 w998 w1006 w1014 w1021 w1027 w1056 w1069 w1098 w1112 w1121 w1129 w1138 w1154 w1185 w1194 w1207 w1222 w1241 w1258 w1274 w1284 w1301 w1335 w1387 w1401 w1414 w1419 w1441 w1447 w1462 w1475 w1506 w1524 w1556 w1577 w1600 w1624 w1635 w1656 w1669 w1689 w1698 w1712 w1718 w1755 w1768 w1789 w1801 w1816 w1830 w1851 w1862 w1874 w1885 w1894 w1903 w1917 w1920 w1926 w1933 w1953 w1961 w1978 w1983 w1987 w1999 w2006 w2023 w2028 w2037 w2042 w2046 w2054 w2068 w2085 w2095 w2113 w2121 w2128 w2136 w2144 w2152 w2162 w2175 w2183 w2194 w2204 w2214 w2222 w2236 w2244 w2252 w2260 w2268 w2276 w2284 w2292 w2300 w2308 w2317 w2328 w2339 w2352 w2362 w2369 w2375 w2426 w2433] -> w27
          tunnel: w21 -> [w33 w726 w735 w750 w764 _ w775 w789 w819 w836 w865 w873 w879 w885 w895 w904 w916 w927 w938 w944 w962 w998 w1006 w1014 w1021 w1027 w1056 w1069 w1098 w1112 w1121 w1129 w1138 w1154 w1184 w1198 w1210 w1228 w1238 w1255 w1267 w1281 w1291 w1316 w1385 w1393 w1406 w1420 w1436 w1446 w1455 w1468 w1506 w1524 w1557 w1564 w1594 w1624 w1635 w1656 w1669 w1689 w1698 w1712 w1717 w1760 w1769 w1789 w1800 w1816 w1829 w1851 w1862 w1874 w1885 w1894 w1903 w1917 w1920 w1926 w1933 w1952 w1961 w1978 w1983 w1988 w2000 w2006 w2018 w2029 w2037 w2042 w2047 w2055 w2069 w2085 w2095 w2113 w2121 w2128 w2136 w2144 w2152 w2162 w2175 w2183 w2194 w2204 w2214 w2222 w2236 w2244 w2252 w2260 w2268 w2276 w2284 w2292 w2300 w2308 w2317 w2328 w2339 w2352 w2362 w2369 w2395 w2426 w2433]
          tunnel: [w36 w727 w733 w752 w755 w771 w776 w799 w820 w837 w866 w874 w881 w886 w900 w910 w923 w928 w940 w947 w963 w999 w1007 w1015 w1022 w1028 w1057 w1070 w1099 w1113 w1122 w1130 w1139 w1155 w1188 w1201 w1212 w1231 w1249 w1264 w1277 w1288 w1305 w1340 w1390 w1404 w1417 w1428 w1444 w1451 w1465 w1482 w1507 w1525 w1559 w1583 w1607 w1625 w1636 w1657 w1670 w1690 w1703 w1713 w1725 w1764 w1775 w1790 w1806 w1817 w1847 w1852 w1863 w1875 w1886 w1895 w1904 w1918 w1924 w1930 w1939 w1956 w1962 w1979 w1984 w1995 w2002 w2007 w2026 w2032 w2039 w2044 w2051 w2063 w2075 w2087 w2097 w2115 w2123 w2130 w2138 w2146 w2154 w2164 w2177 w2185 w2196 w2206 w2216 w2224 w2238 w2246 w2254 w2262 w2270 w2278 w2286 w2294 w2302 w2310 w2319 w2330 w2341 w2354 w2364 w2371 w2398 w2428 w2435] -> w26
          tunnel: [_ _ _ _ _ TRUE _ _ _ _ _ _ _ _ _ _ _ _ _ _ _ _ _ _ _ _ _ _ _ _ _ _ _ _ _ _ _ _ _ _ _ _ _ _ _ _ _ _ _ _ _ _ _ _ _ _ _ _ _ _ _ _ _ _ _ _ _ _ _ _ _ _ _ _ _ _ _ _ _ _ _ _ _ _ _ _ _ _ _ _ _ _ _ _ _ _ _ _ _ _ _ _ _ _ _ _ _ _ _ _ _ _ _ _ _ _ _ _ _ _ _ _ _ _ _ _ _ _ _] -> w25
          tunnel: [w32 w725 w732 w751 w758 w768 w774 w798 w817 w827 w862 w872 w877 w884 w898 w908 w921 w926 w935 w946 w960 w996 w1005 w1013 w1020 w1026 w1039 w1067 w1096 w1104 w1115 w1126 w1136 w1145 w1183 w1197 w1209 w1227 w1246 w1254 w1275 w1286 w1303 w1337 w1388 w1402 w1415 w1426 w1442 w1449 w1463 w1480 w1504 w1521 w1537 w1569 w1605 w1620 w1629 w1654 w1664 w1687 w1701 w1709 w1722 w1762 w1771 w1788 w1804 w1812 w1832 w1850 w1860 w1867 w1884 w1893 w1902 w1916 w1921 w1927 w1932 w1946 w1960 w1967 w1982 w1993 w1998 w2005 w2025 w2031 w2035 w2041 w2048 w2061 w2073 w2084 w2094 w2112 w2120 w2127 w2135 w2143 w2151 w2157 w2174 w2182 w2193 w2203 w2213 w2221 w2235 w2243 w2251 w2259 w2267 w2275 w2283 w2291 w2299 w2307 w2316 w2327 w2338 w2351 w2361 w2368 w2396 w2424 w2431] -> w24
          tunnel: 20 ("Timeout") -> [w31 _ _ _ _ _ _ _ _ _ _ _ _ _ _ _ _ _ _ _ _ _ _ _ _ _ _ _ _ _ _ _ _ _ _ _ _ _ _ _ _ _ _ _ _ _ _ _ _ _ _ _ _ _ _ _ _ _ _ _ _ _ _ _ _ _ _ _ _ _ _ _ _ _ _ _ _ _ _ _ _ _ _ _ _ _ _ _ _ _ _ _ _ _ _ _ _ _ _ _ _ _ _ _ _ _ _ _ _ _ _ _ _ _ _ _ _ _ _ _ _ _ _ _ _ _ _ _ _]
          tunnel: w20 -> [_ _ _ _ _ _ _ w791 _ _ _ _ _ _ _ _ _ _ _ _ _ _ _ _ _ _ _ _ _ _ _ _ _ _ _ _ _ _ _ _ _ _ _ _ _ _ _ _ _ _ _ _ _ _ _ _ _ _ _ _ _ _ _ _ _ _ _ _ _ _ _ _ _ _ _ _ _ _ _ _ _ _ _ _ _ _ _ _ _ _ _ _ _ _ _ _ _ _ _ _ _ _ _ _ _ _ _ _ _ _ _ _ _ _ _ _ _ _ _ _ _ _ _ _ _ _ _ _ _]
          tunnel: [w30 w724 w729 w741 w766 w769 w773 w797 w818 w835 w864 w871 w876 w883 w899 w909 w922 w925 w939 w945 w957 w997 w1004 w1012 w1019 w1025 w1055 w1068 w1097 w1111 w1120 w1128 w1137 w1153 w1187 w1200 w1211 w1230 w1248 w1263 w1276 w1287 w1304 w1339 w1389 w1403 w1416 w1427 w1443 w1450 w1464 w1481 w1505 w1523 w1558 w1582 w1606 w1623 w1634 w1655 w1668 w1688 w1702 w1711 w1724 w1763 w1774 w1787 w1805 w1815 w1846 w1849 w1861 w1873 w1883 w1892 w1901 w1915 w1923 w1929 w1938 w1955 w1959 w1973 w1981 w1994 w2001 w2004 w2024 w2030 w2038 w2043 w2050 w2062 w2074 w2086 w2096 w2114 w2122 w2129 w2137 w2145 w2153 w2163 w2176 w2184 w2195 w2205 w2215 w2223 w2237 w2245 w2253 w2261 w2269 w2277 w2285 w2293 w2301 w2309 w2318 w2329 w2340 w2353 w2363 w2370 w2397 w2427 w2434] -> w19
          tunnel: w18 -> [w30 w724 w729 w741 w766 w769 w773 w797 w818 w835 w864 w871 w876 w883 w899 w909 w922 w925 w939 w945 w957 w997 w1004 w1012 w1019 w1025 w1055 w1068 w1097 w1111 w1120 w1128 w1137 w1153 w1187 w1200 w1211 w1230 w1248 w1263 w1276 w1287 w1304 w1339 w1389 w1403 w1416 w1427 w1443 w1450 w1464 w1481 w1505 w1523 w1558 w1582 w1606 w1623 w1634 w1655 w1668 w1688 w1702 w1711 w1724 w1763 w1774 w1787 w1805 w1815 w1846 w1849 w1861 w1873 w1883 w1892 w1901 w1915 w1923 w1929 w1938 w1955 w1959 w1973 w1981 w1994 w2001 w2004 _ w2030 w2038 w2043 w2050 w2062 w2074 w2086 w2096 w2114 w2122 w2129 w2137 w2145 w2153 w2163 w2176 w2184 w2195 w2205 w2215 w2223 w2237 w2245 w2253 w2261 w2269 w2277 w2285 w2293 w2301 w2309 w2318 w2329 w2340 w2353 w2363 w2370 w2397 w2427 w2434]
          frame "", "Idle" {
            # "executes when the state queue is empty"
            n8 = event shown="[34] \"Remove Offset\": Value Change" {
              selector: w30 -> [_ _ _ _ _ _ _ _ _ _ _ _ _ _ _ _ _ _ _ _ _ _ _ _ _ _ _ _ _ _ _ _ _ _ _ _ _ _ _ _ _ _ _ _ _ _ _ _ _ _ _ _ _ _ _ _ _ _ _ _ _ _ _ _ _ _ _ _ _ _ _ _ _ _ _ _]
              dyn-events: _ -> [_ _ _ _ _ _ _ _ _ _ _ _ _ _ _ _ _ _ _ _ _ _ _ _ _ _ _ _ _ _ _ _ _ _ _ _ _ _ _ _ _ _ _ _ _ _ _ _ _ _ _ _ _ _ _ _ _ _ _ _ _ _ _ _ _ _ _ _ _ _ _ _ _ _ _ _]
              timeout: w31 -> [_ _ _ _ _ _ _ _ _ _ _ _ _ _ _ _ _ _ _ _ _ _ _ _ _ _ _ _ _ _ _ _ _ _ _ _ _ _ _ _ _ _ _ _ _ _ _ _ _ _ _ _ _ _ _ _ _ _ _ _ _ _ _ _ _ _ _ _ _ _ _ _ _ _ _ _]
              tunnel: w37 -> [w51 w89 w97 w111 w115 w126 w134 w149 w157 w165 w169 w175 w182 w188 w199 w218 w231 w238 w245 w253 w271 w288 w295 w302 w309 w316 w323 w331 w339 w347 w355 w361 w370 w386 w399 w407 w415 w423 w430 w437 w441 w446 w451 w456 w461 w466 w475 w489 w503 w515 w527 w542 w547 w552 w557 w562 w566 w571 w576 w580 w584 w590 w606 w621 w634 w641 w648 w655 w662 w669 w686 w693 w702 w709 w716 w723]
              tunnel: [w50 w88 w96 w110 w114 w125 w133 w148 w156 w164 w168 w174 w181 w187 w198 w217 w230 w237 w244 w252 w270 w287 w294 w301 w308 w315 w322 w330 w338 w346 w354 w360 w369 w385 w398 w406 w414 w422 w429 w436 w440 w445 w450 w455 w460 w465 w474 w488 w502 w514 w526 w541 w546 w551 w556 w561 w565 w570 w575 w579 w583 w589 w605 w620 w633 w640 w647 w654 w661 w668 w685 w692 w701 w708 w715 w722] -> w36
              tunnel: w35 -> [w48 w86 w94 w108 w113 w118 w127 w137 w150 w159 w167 w170 w177 w183 w195 w209 w226 w233 w239 w246 w262 w283 w290 w297 w304 w311 w318 w326 w334 w342 w350 w356 w365 w373 w392 w400 w411 w419 w427 w434 w439 w442 w447 w452 w457 w462 w470 w486 w500 w512 w524 w539 w544 w550 w554 w559 w564 w568 w573 w577 w581 w587 w598 w615 w627 w636 w644 w650 w658 w664 w678 w688 w697 w704 w711 w718]
              tunnel: [w49 w87 w93 w107 w112 w123 w131 w146 w154 w162 w166 w171 w179 w186 w197 w212 w229 w236 w243 w251 w269 w285 w292 w299 w306 w313 w320 w328 w336 w344 w352 w357 w367 w383 w396 w404 w412 w420 w428 w435 w438 w443 w448 w453 w458 w463 w472 w487 w501 w513 w525 w540 w543 w549 w553 w558 w563 w569 w574 w578 w582 w588 w604 w619 w630 w639 w646 w653 w660 w667 w684 w691 w700 w707 w714 w721] -> w34
              tunnel: w33 -> [w49 w87 w92 w107 w112 w123 w131 w146 w154 w162 w166 w171 w179 w186 w197 w212 w229 w236 w243 w251 w269 w285 w292 w299 w306 w313 w320 w328 w336 w344 w352 w357 w367 w383 w396 w404 w412 w420 w428 w435 w438 w443 w448 w453 w458 w463 w472 w487 w501 w513 w525 w540 w543 w549 w553 w558 w563 w569 w574 w578 w582 w588 w604 w619 w630 w639 w646 w653 w660 w667 w684 w691 w700 w707 w714 w721]
              tunnel: [w48 w86 w94 w108 w113 w119 w127 w136 w150 w159 w167 w170 w178 w185 w196 w211 w228 w235 w242 w250 w261 w284 w291 w298 w305 w312 w319 w327 w335 w343 w351 w356 w366 w382 w392 w400 w411 w419 w427 w434 w439 w442 w447 w452 w457 w462 w471 w486 w500 w512 w524 w539 w544 w550 w554 w559 w564 w568 w573 w577 w581 w587 w603 w614 w632 w637 w645 w652 w659 w665 w683 w689 w698 w705 w712 w719] -> w32
              event Timeout {
                n9 = event-data() -> ()  [unwired: 1 in, 1 out]
                n10 = Unbundle By Name(w48) -> ("DAQ state"=w47:T33)
                n11 = call <userlib>:"Periodic Trigger__ogtk.vi"("time (ms)"=u32 100) -> ("Triggered"=w45:bool)  [unwired: 12 in, 2 out]
                n12 = call <userlib>:"Periodic Trigger__ogtk.vi"("time (ms)"=u32 600000) -> ("Triggered"=w42:bool)  [unwired: 12 in, 2 out]
                n13 = case shown="True" w45 {
                  tunnel: w47 -> [_ w57]
                  tunnel: [w54 w56] -> w40
                  tunnel: [w54 "idle"] -> w38
                  frame False {
                    w54 = "" ("States Out")
                  }
                  frame True {
                    n14 = case shown="\"started\"" w57 {
                      tunnel: [w58 w64 w72 w76 ""] -> w56
                      frame "idle" {
                        n15 = call "Spinner.vi"("Enum"=T28."Spinner 1") -> ("Spinner Out"=w61:string)  [unwired: 4 in]
                        n16 = Concatenate Strings("Idle     " ("Status"), w61) -> (w59:string)
                        n17 = call <vilib>:"Build State String with Arguments__JKI_lib_State_Machine.vi"("Arguments (\"\")"=w59, "State"="UI: Update Status") -> ("State with Arguments"=w58:string)  [unwired: 4 in]
                      }
                      frame "created" {
                        n18 = call "Spinner.vi"("Enum"=T28."Spinner 1") -> ("Spinner Out"=w67:string)  [unwired: 4 in]
                        n19 = Concatenate Strings("Created  " ("Status"), w67) -> (w65:string)
                        n20 = call <vilib>:"Build State String with Arguments__JKI_lib_State_Machine.vi"("Arguments (\"\")"=w65, "State"="UI: Update Status") -> ("State with Arguments"=w64:string)  [unwired: 4 in]
                      }
                      frame "started" {
                        n21 = call "Spinner3.vi"("String In"="OK") -> ("Spinner Out"=w70:string)  [unwired: 4 in]
                        n22 = call <vilib>:"Build State String with Arguments__JKI_lib_State_Machine.vi"("Arguments (\"\")"=w70, "State"="UI: Update Status") -> ("State with Arguments"=w72:string)  [unwired: 4 in]
                      }
                      frame "sweeping" {
                        n23 = call "Spinner2.vi"("String In"="sweeping") -> ("Spinner Out"=w74:string)  [unwired: 4 in]
                        n24 = call <vilib>:"Build State String with Arguments__JKI_lib_State_Machine.vi"("Arguments (\"\")"=w74, "State"="UI: Update Status") -> ("State with Arguments"=w78:string)  [unwired: 4 in]
                        n25 = call <vilib>:"Add State(s) to Queue__jki_lib_state_machine.vi"("State(s) in Front (\"\")"=w78, "State(s) at Back (\"\")"="UI: Update Sweep Timer") -> ("States Out"=w76:string)  [unwired: 13 in]
                      }
                      frame Default {
                      }
                    }
                  }
                }
                n26 = case shown="True" w42 {
                  tunnel: ["" "Macro: Save Configuration"] -> w41
                  frame False {
                  }
                  frame True {
                    # "Backup configuration every 10 minutes"
                  }
                }
                n27 = call <userlib>:"MGI Milliseconds Since Last Call.vi"() -> ("ms"=→"UI Refresh Time (ms)":u32)  [unwired: 6 in, 1 out]
                n28 = call <vilib>:"Add State(s) to Queue__jki_lib_state_machine.vi"("State(s) in Front (\"\")"=w40, "State(s) in (\"\")"=w38, "State(s) at Back (\"\")"=w41) -> ("States Out"=w39:string)  [unwired: 12 in]
                n29 = call <vilib>:"Add State(s) to Queue__jki_lib_state_machine.vi"("State(s) in Front (\"\")"=w39, "State(s) in (\"\")"=w51) -> ("States Out"=w50:string)  [unwired: 13 in]
              }
              event "Close": Value Change {
                # "Hide this FP control 2022-08-15"
                n30 = event-data() -> ()  [unwired: 1 in, 6 out]
                n31 = Two Button Dialog(message="Are you sure you want to stop this program?") -> (T button?=w81:bool)  [unwired: 2 in]
                n32 = Select(t="Action: Notify UI Closed\nMacro: Exit", s=w81, f="") -> (s? t:f=w82:string)
                n33 = local write "Close"(w81) -> ()
                n34 = call <vilib>:"Add State(s) to Queue__jki_lib_state_machine.vi"("State(s) in Front (\"\")"=w82, "State(s) in (\"\")"=w89) -> ("States Out"=w88:string)  [unwired: 13 in]
              }
              event "Help": Value Change {
                # "HELP Value Change Event (Button Pressed)\n(If Help = True: Send user to help webpage; Set Help=False\nIf Help=False, Do nothing)"
                n35 = event-data() -> ("NewVal"=w91:bool)  [unwired: 1 in, 5 out]
                n36 = local write "Help"(FALSE ("Help")) -> ()
                n37 = case shown="True" w91 {
                  tunnel: w92 -> [w98 w101]
                  tunnel: [w98 w100] -> w93
                  frame False {
                  }
                  frame True {
                    n38 = call-poly <vilib>:"Open URL in Default Browser.vi"("error in (no error)"=w101, "URL"="https://github.com/levylabpitt/Multichannel-Lockin") -> ("error out"=w100:errorcluster)  [unwired: 4 in, 1 out]
                  }
                }
                n39 = call <vilib>:"Add State(s) to Queue__jki_lib_state_machine.vi"("State(s) in Front (\"\")"="", "State(s) in (\"\")"=w97) -> ("States Out"=w96:string)  [unwired: 13 in]
              }
              event Panel Close? {
                # "Discard the event because we'll close the front panel ourselves in Macro: Exit"
                # "Close Panel button (pressed) Event\n(this executes Macro: Exit to terminate the VI)"
                n40 = event-data() -> ()  [unwired: 1 in, 1 out]
                n41 = Two Button Dialog(message="Are you sure you want to stop this program?") -> (T button?=w106:bool)  [unwired: 2 in]
                n42 = Select(t="Action: Notify UI Closed\nMacro: Exit", s=w106, f="") -> (s? t:f=w102:string)
                n43 = event-data("Discard?"=TRUE) -> ()  [unwired: 1 in, 1 out]
                n44 = call <vilib>:"Add State(s) to Queue__jki_lib_state_machine.vi"("State(s) in Front (\"\")"=w102, "State(s) in (\"\")"=w111) -> ("States Out"=w110:string)  [unwired: 13 in]
              }
              event "....................State....................": Value Change {
                # "Do not put any code in this frame.\n(it is a separator no-op)"
                n45 = event-data() -> ()  [unwired: 1 in, 6 out]
                n46 = call <vilib>:"Add State(s) to Queue__jki_lib_state_machine.vi"("State(s) in (\"\")"=w115) -> ("States Out"=w114:string)  [unwired: 14 in]
              }
              event "Start": Value Change {
                w116 = TRUE ("update graphs")
                w117 = T43 10123 items=["Finite Samples"=10178, "Continuous Samples"=10123] ("UI Config.DAQ.Sampling.Sample Mode")
                # "Start Button Change Event (Button Pressed)\n()"
                n47 = event-data() -> ()  [unwired: 1 in, 6 out]
                n48 = local write "Start"(FALSE ("Help")) -> ()
                n49 = Bundle By Name(cluster=w118, "UI Config.DAQ.cfg.Sampling.sample mode"=w117, "update waveform graphs"=w116, "update lockin graphs"=w116) -> (w119:T65)
                n50 = Format Into String(format string="Action: Sampling\nAction: Command\nAction: State >> %s\nAction: Command", State--enum."start" ("State")) -> (resulting string=w120:string)  [unwired: 2 in, 1 out]
                n51 = call <vilib>:"Add State(s) to Queue__jki_lib_state_machine.vi"("State(s) in Front (\"\")"=w120, "State(s) in (\"\")"=w126) -> ("States Out"=w125:string)  [unwired: 13 in]
              }
              event "Pause": Value Change {
                # "Start Button Change Event (Button Pressed)\n()"
                n52 = event-data() -> ()  [unwired: 1 in, 6 out]
                n53 = local write "Pause"(FALSE ("Help")) -> ()
                n54 = Format Into String(format string="Action: State >> %s\nAction: Command\nMacro: Save Configuration", State--enum."stop" ("State")) -> (resulting string=w128:string)  [unwired: 2 in, 1 out]
                n55 = call <vilib>:"Add State(s) to Queue__jki_lib_state_machine.vi"("State(s) in Front (\"\")"=w128, "State(s) in (\"\")"=w134) -> ("States Out"=w133:string)  [unwired: 13 in]
              }
              event "Reset": Value Change {
                w135 = TRUE
                # "Start Button Change Event (Button Pressed)\n()"
                n56 = event-data() -> ()  [unwired: 1 in, 6 out]
                n57 = local write "Reset"(FALSE ("Help")) -> ()
                n58 = Format Into String(format string="Action: State >> %s\nAction: Command\nMacro: Save Configuration", State--enum."stop" ("State")) -> (resulting string=w141:string)  [unwired: 2 in, 1 out]
                n59 = Format Into String(format string="Action: State >> %s\nAction: Command", State--enum."start" ("State")) -> (resulting string=w139:string)  [unwired: 2 in, 1 out]
                n60 = Bundle By Name(cluster=w137, "update waveform graphs"=w135, "update lockin graphs"=w135) -> (w136:T65)
                n61 = call <vilib>:"Add State(s) to Queue__jki_lib_state_machine.vi"("State(s) in Front (\"\")"=w141, "State(s) in (\"\")"="Action: Sampling\nAction: Command\nData: Wait >> 250", "State(s) at Back (\"\")"=w139) -> ("States Out"=w138:string)  [unwired: 12 in]
                n62 = call <vilib>:"Add State(s) to Queue__jki_lib_state_machine.vi"("State(s) in Front (\"\")"=w138, "State(s) in (\"\")"=w149) -> ("States Out"=w148:string)  [unwired: 13 in]
              }
              event "Start Sweep": Value Change {
                # "Stop Sweep Value Change Event (Button Pressed)\n()"
                n63 = event-data() -> ()  [unwired: 1 in, 6 out]
                n64 = local write "Start Sweep"(FALSE ("Help")) -> ()
                n65 = Format Into String(format string="Action: State >> %s\nAction: Command", State--enum."start sweep" ("State")) -> (resulting string=w152:string)  [unwired: 2 in, 1 out]
                n66 = call <vilib>:"Add State(s) to Queue__jki_lib_state_machine.vi"("State(s) in Front (\"\")"=w152, "State(s) in (\"\")"=w157) -> ("States Out"=w156:string)  [unwired: 13 in]
              }
              event "Stop Sweep": Value Change {
                # "Stop Sweep Value Change Event (Button Pressed)\n()"
                n67 = event-data() -> ()  [unwired: 1 in, 6 out]
                n68 = local write "Stop Sweep"(FALSE ("Help")) -> ()
                n69 = Format Into String(format string="Action: State >> %s\nAction: Command\nMacro: Save Configuration", State--enum."stop sweep" ("State")) -> (resulting string=w158:string)  [unwired: 2 in, 1 out]
                n70 = call <vilib>:"Add State(s) to Queue__jki_lib_state_machine.vi"("State(s) in Front (\"\")"=w158, "State(s) in (\"\")"=w165) -> ("States Out"=w164:string)  [unwired: 13 in]
              }
              event "....................DAQ and Channel....................": Value Change {
                # "Do not put any code in this frame.\n(it is a separator no-op)"
                n71 = event-data() -> ()  [unwired: 1 in, 6 out]
                n72 = call <vilib>:"Add State(s) to Queue__jki_lib_state_machine.vi"("State(s) in (\"\")"=w169) -> ("States Out"=w168:string)  [unwired: 14 in]
              }
              event "Auto DAQ": Value Change {
                # "auto DAQ Value Change Event (Button Pressed)\n()"
                n73 = event-data() -> ()  [unwired: 1 in, 6 out]
                n74 = local write "Auto DAQ"(FALSE ("Help")) -> ()
                n75 = call <vilib>:"Add State(s) to Queue__jki_lib_state_machine.vi"("State(s) in Front (\"\")"="Action: Auto DAQ\nAction: Command", "State(s) in (\"\")"=w175) -> ("States Out"=w174:string)  [unwired: 13 in]
              }
              event Value Change {
                # "DAQ Config Value Change Event (Button Pressed)\n()"
                n76 = event-data() -> ()  [unwired: 1 in, 6 out]
                n77 = Bundle By Name(cluster=w177, "UI Config.DAQ.Configuration"="DAQ Config") -> (w178:T65)
                n78 = call <vilib>:"Add State(s) to Queue__jki_lib_state_machine.vi"("State(s) in Front (\"\")"="Action: DAQ Config\nAction: Command", "State(s) in (\"\")"=w182) -> ("States Out"=w181:string)  [unwired: 13 in]
              }
              event "Fs (S/s)", "#s (S)": Value Change {
                # "DAQ Config Value Change Event (Button Pressed)\n()"
                n79 = event-data() -> ()  [unwired: 1 in, 6 out]
                n80 = disable-structure shown="Disabled" {
                  disable-tunnel: [w192 w193] -> w185
                  disable-tunnel: ["Action: Sampling\nAction: Command" _] -> w184
                  disable-tunnel: w183 -> [w190 w193]
                  frame Disabled {
                    n81 = local read "Fs Output (S/s)"() -> (w189:dbl)
                    n82 = Bundle By Name(cluster=w190) -> (w192:T65)  [unwired: 2 in]
                    n83 = property on="Fs Output (S/s)" class="DigNum (strict)"("Val(Sgnl)"=w189) -> ()  [unwired: 2 in, 2 out]
                  }
                  frame Enabled {
                  }
                }
                n84 = call <vilib>:"Add State(s) to Queue__jki_lib_state_machine.vi"("State(s) in Front (\"\")"=w184, "State(s) in (\"\")"=w188) -> ("States Out"=w187:string)  [unwired: 13 in]
              }
              event "Fs Output (S/s)": Value Change {
                # "DAQ Config Value Change Event (Button Pressed)\n()"
                n85 = event-data() -> ()  [unwired: 1 in, 6 out]
                n86 = disable-structure shown="Disabled" {
                  disable-tunnel: [w206 w207] -> w196
                  disable-tunnel: w195 -> [w205 w207]
                  disable-tunnel: ["Action: Sampling Fs Output\nAction: Command" _] -> w194
                  frame Disabled {
                    n87 = Unbundle By Name(w205) -> ("UI Config.DAQ.cfg.Sampling.Sampling.Fs"=w203:dbl, "UI Config.DAQ.cfg.Sampling.Sampling.#s"=w204:i32)
                    n88 = Divide(x=w203, y=w204) -> (x/y=w202:dbl)
                    n89 = In Range and Coerce(upper limit=w203, lower limit=w202) -> (coerced(x)=w201:dbl)  [unwired: 1 in, 1 out]
                    n90 = local write "Fs Output (S/s)"(w201) -> ()
                    n91 = Bundle By Name(cluster=w205, "UI Config.DAQ.cfg.Sampling.Fs.Output"=w201) -> (w206:T65)
                  }
                  frame Enabled {
                  }
                }
                n92 = call <vilib>:"Add State(s) to Queue__jki_lib_state_machine.vi"("State(s) in Front (\"\")"=w194, "State(s) in (\"\")"=w199) -> ("States Out"=w198:string)  [unwired: 13 in]
              }
              event Value Change {
                n93 = event-data() -> ()  [unwired: 1 in, 6 out]
                n94 = control-ref of="Fs Multiplier"() -> (w216:refnum<vi>)
                n95 = control-ref of="Refresh Rate (Hz)"() -> (w215:refnum<vi>)
                n96 = Bundle By Name(cluster=w209, "UI Config.DAQ.cfg.Sampling.Fs Mode"="Fs Mode") -> (w211:T65)
                n97 = case shown="\"Manual\"" "Fs Mode" {
                  tunnel: [FALSE ("Visible") TRUE ("Visible") FALSE ("Visible")] -> w214
                  tunnel: [FALSE ("Visible") FALSE ("Visible") TRUE ("Visible")] -> w213
                  frame "Manual" {
                  }
                  frame "Auto Fs" {
                  }
                  frame "Max Fs" {
                  }
                }
                n98 = property class="DigNum (strict)"(reference=w216, "Visible"=w214) -> ()  [unwired: 1 in, 2 out]
                n99 = property class="DigNum (strict)"(reference=w215, "Visible"=w213) -> ()  [unwired: 1 in, 2 out]
                n100 = call <vilib>:"Add State(s) to Queue__jki_lib_state_machine.vi"("State(s) in Front (\"\")"="Action: Sampling Fs Mode\nAction: Command", "State(s) in (\"\")"=w218) -> ("States Out"=w217:string)  [unwired: 13 in]
              }
              event "Fs Multiplier": Value Change {
                # "DAQ Config Value Change Event (Button Pressed)\n()"
                n101 = event-data() -> ()  [unwired: 1 in, 6 out]
                n102 = Bundle By Name(cluster=w226, "UI Config.DAQ.cfg.Sampling.Fs Multiplier"="Fs Multiplier") -> (w228:T65)
                n103 = call <vilib>:"Add State(s) to Queue__jki_lib_state_machine.vi"("State(s) in Front (\"\")"="Action: Sampling Fs Multiplier\nAction: Command", "State(s) in (\"\")"=w231) -> ("States Out"=w230:string)  [unwired: 13 in]
              }
              event "Refresh Rate (Hz)": Value Change {
                # "DAQ Config Value Change Event (Button Pressed)\n()"
                n104 = event-data() -> ()  [unwired: 1 in, 6 out]
                n105 = Bundle By Name(cluster=w233, "UI Config.DAQ.cfg.Sampling.Refresh Rate (Hz)"="Refresh Rate (Hz)") -> (w235:T65)
                n106 = call <vilib>:"Add State(s) to Queue__jki_lib_state_machine.vi"("State(s) in Front (\"\")"="Action: Sampling Refresh Rate\nAction: Command", "State(s) in (\"\")"=w238) -> ("States Out"=w237:string)  [unwired: 13 in]
              }
              event "Decimation (pre DSP)": Value Change {
                # "Decimation Value Change Event (Button Pressed)\n()"
                n107 = event-data() -> ()  [unwired: 1 in, 6 out]
                n108 = Bundle By Name(cluster=w239, "UI Config.DAQ.cfg.Sampling.Decimation.PreDSP"="Decimation (pre DSP)") -> (w242:T65)
                n109 = call <vilib>:"Add State(s) to Queue__jki_lib_state_machine.vi"("State(s) in Front (\"\")"="Action: Sampling Decimation Pre DSP\nAction: Command", "State(s) in (\"\")"=w245) -> ("States Out"=w244:string)  [unwired: 13 in]
              }
              event "Decimation (post DSP)": Value Change {
                # "hide from user for now (8/12/2022)"
                # "Decimation Value Change Event (Button Pressed)\n()"
                n110 = event-data() -> ()  [unwired: 1 in, 6 out]
                n111 = Unbundle By Name(w246) -> ("DAQ state"=w248:T33)
                n112 = Bundle By Name(cluster=w246, "UI Config.DAQ.cfg.Sampling.Decimation.PostDSP"="Decimation (post DSP)") -> (w250:T65)
                n113 = case shown="\"started\"" w248 {
                  tunnel: ["Action: Sampling Decimation Post DSP\nAction: Command" w256] -> w247
                  frame Default {
                  }
                  frame "started" {
                    n114 = Format Into String(format string="Action: State >> %s\nAction: Command\nAction: Sampling Decimation Post DSP\nAction: Command\nAction: State >> %s\nAction: Command", State--enum."stop" ("State"), State--enum."start" ("State")) -> (resulting string=w256:string)  [unwired: 2 in, 1 out]
                  }
                }
                n115 = call <vilib>:"Add State(s) to Queue__jki_lib_state_machine.vi"("State(s) in Front (\"\")"=w247, "State(s) in (\"\")"=w253) -> ("States Out"=w252:string)  [unwired: 13 in]
              }
              event Value Change {
                # "check if ref index changed"
                # "AI Channels Value Change Event (Button Pressed)\n()"
                n116 = event-data() -> ("OldVal"=w268:T4, "NewVal"=w264:T4)  [unwired: 1 in, 4 out]
                n117 = Not Equal?(x=w268, y=w264) -> (x != y?=w267:T66)
                n118 = for {
                  tunnel: w267 -> [w281] mode=indexing
                  tunnel: [w280] -> w266 mode=indexing
                  n119 = Unbundle By Name(w281) -> ("reference index"=w280:bool)
                }
                n120 = Search 1D Array(1D array=w266, element=TRUE) -> (index of element=w263:i32)  [unwired: 1 in]
                n121 = case shown="-1" w263 {
                  selector: w263 -> [_ w278]
                  tunnel: w262 -> [w275 w279]
                  tunnel: [w274 w279] -> w261
                  tunnel: ["Action: AI Channels\nAction: Command" w276] -> w260
                  tunnel: "AI Channels" -> [w272 _]
                  frame -1 {
                    # "something else changed, alert DAQ process"
                    n122 = Bundle By Name(cluster=w275, "UI Config.Channels.Cfg_AI"=w272) -> (w274:T65)
                  }
                  frame Default {
                    n123 = Format Into String(format string="UI: Sync AI Ref Array >> %d", w278) -> (resulting string=w276:string)  [unwired: 2 in, 1 out]
                  }
                }
                n124 = call <vilib>:"Add State(s) to Queue__jki_lib_state_machine.vi"("State(s) in Front (\"\")"=w260, "State(s) in (\"\")"=w271) -> ("States Out"=w270:string)  [unwired: 13 in]
              }
              event Value Change {
                # "AO Channels Value Change Event (Button Pressed)\n()"
                n125 = event-data() -> ()  [unwired: 1 in, 6 out]
                n126 = Bundle By Name(cluster=w283, "UI Config.Channels.Cfg_AO"="AO Channels") -> (w284:T65)
                n127 = call <vilib>:"Add State(s) to Queue__jki_lib_state_machine.vi"("State(s) in Front (\"\")"="Action: AO Channels\nAction: Command", "State(s) in (\"\")"=w288) -> ("States Out"=w287:string)  [unwired: 13 in]
              }
              event Value Change {
                # "REF Channels Value Change Event (Button Pressed)\n()"
                n128 = event-data() -> ()  [unwired: 1 in, 6 out]
                n129 = Bundle By Name(cluster=w290, "UI Config.Channels.Cfg_REF"="REF Channels") -> (w291:T65)
                n130 = call <vilib>:"Add State(s) to Queue__jki_lib_state_machine.vi"("State(s) in Front (\"\")"="Action: REF Channels\nAction: Command\nAction: Sampling Fs Output\nAction: Command", "State(s) in (\"\")"=w295) -> ("States Out"=w294:string)  [unwired: 13 in]
              }
              event Value Change {
                # "DAQ Config Value Change Event (Button Pressed)\n()"
                n131 = event-data() -> ()  [unwired: 1 in, 6 out]
                n132 = Bundle By Name(cluster=w297, "UI Config.DAQ.Simulation mode"="AI Simulation mode") -> (w298:T65)
                n133 = call <vilib>:"Add State(s) to Queue__jki_lib_state_machine.vi"("State(s) in Front (\"\")"="Action: AI Simulate Mode\nAction: Command", "State(s) in (\"\")"=w302) -> ("States Out"=w301:string)  [unwired: 13 in]
              }
              event Value Change {
                # "DAQ Config Value Change Event (Button Pressed)\n()"
                n134 = event-data() -> ()  [unwired: 1 in, 6 out]
                n135 = Bundle By Name(cluster=w304, "UI Config.Amplifers.Gain_AI"="Input Gain") -> (w305:T65)
                n136 = call <vilib>:"Add State(s) to Queue__jki_lib_state_machine.vi"("State(s) in Front (\"\")"="Action: Input Gain\nAction: Command", "State(s) in (\"\")"=w309) -> ("States Out"=w308:string)  [unwired: 13 in]
              }
              event Value Change {
                # "DAQ Config Value Change Event (Button Pressed)\n()"
                n137 = event-data() -> ()  [unwired: 1 in, 6 out]
                n138 = Bundle By Name(cluster=w311, "UI Config.Amplifers.Offset_AI"="Input Offsets") -> (w312:T65)
                n139 = call <vilib>:"Add State(s) to Queue__jki_lib_state_machine.vi"("State(s) in Front (\"\")"="Action: Offset\nAction: Command", "State(s) in (\"\")"=w316) -> ("States Out"=w315:string)  [unwired: 13 in]
              }
              event Value Change {
                # "DAQ Config Value Change Event (Button Pressed)\n()"
                n140 = event-data() -> ()  [unwired: 1 in, 6 out]
                n141 = Bundle By Name(cluster=w318, "UI Config.Amplifers.Gain_AO"="Output Gain") -> (w319:T65)
                n142 = call <vilib>:"Add State(s) to Queue__jki_lib_state_machine.vi"("State(s) in Front (\"\")"="Action: Output Gain\nAction: Command", "State(s) in (\"\")"=w323) -> ("States Out"=w322:string)  [unwired: 13 in]
              }
              event "AC Limit", "Limit AC?": Value Change {
                # "Limit Amplitudes Paramaters Change Event ()\n()"
                n143 = event-data() -> ()  [unwired: 1 in, 6 out]
                n144 = Bundle By Name(cluster=w326, "UI Config.Limit Amplitude.Limit?"="Limit AC?", "UI Config.Limit Amplitude.Limit (V)"="AC Limit") -> (w327:T65)
                n145 = call <vilib>:"Add State(s) to Queue__jki_lib_state_machine.vi"("State(s) in Front (\"\")"="Action: Limit Amplitude\nAction: Command", "State(s) in (\"\")"=w331) -> ("States Out"=w330:string)  [unwired: 13 in]
              }
              event "AO DC Limit", "Limit DC?": Value Change {
                # "Limit Amplitudes Paramaters Change Event ()\n()"
                n146 = event-data() -> ()  [unwired: 1 in, 6 out]
                n147 = Bundle By Name(cluster=w334, "UI Config.Limit DC.Limit?"="Limit DC?", "UI Config.Limit DC.Limit (V)"="AO DC Limit") -> (w335:T65)
                n148 = call <vilib>:"Add State(s) to Queue__jki_lib_state_machine.vi"("State(s) in Front (\"\")"="Action: Limit DC\nAction: Command", "State(s) in (\"\")"=w339) -> ("States Out"=w338:string)  [unwired: 13 in]
              }
              event "Link f?", "f link (Hz)": Value Change {
                # "Link Frequencies Parameters Change Event ()\n()"
                n149 = event-data() -> ()  [unwired: 1 in, 6 out]
                n150 = Bundle By Name(cluster=w342, "UI Config.Link Frequencies.Link?"="Link f?", "UI Config.Link Frequencies.Frequency (Hz)"="f link (Hz)") -> (w343:T65)
                n151 = call <vilib>:"Add State(s) to Queue__jki_lib_state_machine.vi"("State(s) in Front (\"\")"="Action: Link Frequencies\nAction: Command", "State(s) in (\"\")"=w347) -> ("States Out"=w346:string)  [unwired: 13 in]
              }
              event "duty cycle (%)": Value Change {
                # "Link Frequencies Parameters Change Event ()\n()"
                n152 = event-data() -> ()  [unwired: 1 in, 6 out]
                n153 = Bundle By Name(cluster=w350, "UI Config.Function Option.Option?"=FALSE ("Function Option"), "UI Config.Function Option.Duty Cycle (%)"="duty cycle (%)") -> (w351:T65)
                n154 = call <vilib>:"Add State(s) to Queue__jki_lib_state_machine.vi"("State(s) in Front (\"\")"="Action: Duty Cycle\nAction: Command", "State(s) in (\"\")"=w355) -> ("States Out"=w354:string)  [unwired: 13 in]
              }
              event "Reset Phase": Value Change {
                # "Reset Phase Value Change Event (Button Pressed)\n()"
                n155 = event-data() -> ()  [unwired: 1 in, 6 out]
                n156 = local write "Reset Phase"(FALSE ("Help")) -> ()
                n157 = call <vilib>:"Add State(s) to Queue__jki_lib_state_machine.vi"("State(s) in Front (\"\")"="Action: Zero Phase\nAction: Command", "State(s) in (\"\")"=w361) -> ("States Out"=w360:string)  [unwired: 13 in]
              }
              event "Line", "Lowpass", "LP f (Hz)": Value Change {
                # "Prefilter Paramters Change Event ()\n()"
                n158 = event-data() -> ()  [unwired: 1 in, 6 out]
                n159 = Bundle By Name(cluster=w365, "UI Config.PreFilter.60 Hz"="Line", "UI Config.PreFilter.Low Pass"="Lowpass", "UI Config.PreFilter.Low Pass Cutoff (Hz)"="LP f (Hz)") -> (w366:T65)
                n160 = call <vilib>:"Add State(s) to Queue__jki_lib_state_machine.vi"("State(s) in Front (\"\")"="Action: PreFilter\nAction: Command", "State(s) in (\"\")"=w370) -> ("States Out"=w369:string)  [unwired: 13 in]
              }
              event "Sweep Time (s)", "Return to Start?", "Initial Wait (s)", "Sweep Pattern": Value Change {
                # "Sweep Parameters (Time, Wait, Return, Channels) Change Event ()\n()"
                n161 = event-data() -> ()  [unwired: 1 in, 6 out]
                n162 = Unbundle By Name(w373) -> ("UI Config.Sweep"=w378:T55)
                n163 = for {
                  tunnel: [w391] -> w371 mode=indexing
                  tunnel: "Sweep Pattern" -> [w390] mode=indexing
                  n164 = Unbundle By Name(w390) -> ("Channel"=w389:u16, "Sweep Pattern"=w388:dbl[])
                  n165 = Bundle By Name(cluster=T30 {"Channel"=1, "Table"=[]} ("setSweep_Table"), "Channel"=w389, "Table"=w388) -> (w391:T30)
                }
                n166 = Bundle By Name(cluster=w378, "sweepTime"="Sweep Time (s)", "initialWaitTime"="Initial Wait (s)", "returnToStart"="Return to Start?", "sweepChannels"="Sweep Channels") -> (w372:T55)
                n167 = call "Replace Sweep Waveforms.vi"("Channels New"=w371, "Sweep in"=w372) -> ("Sweep out"=w379:T55)  [unwired: 9 in]
                n168 = Bundle By Name(cluster=w373, "UI Config.Sweep"=w379) -> (w382:T65)
                n169 = call <vilib>:"Add State(s) to Queue__jki_lib_state_machine.vi"("State(s) in Front (\"\")"="Action: Sweep\nAction: Command", "State(s) in (\"\")"=w386) -> ("States Out"=w385:string)  [unwired: 13 in]
                "Sweep Timer (s)" <- 0.0 ("Sweep Timer (s)")
              }
              event "Remove Offset": Value Change {
                # "Remove Offset Value Change Event (Button Pressed)\n()"
                n170 = event-data() -> ()  [unwired: 1 in, 6 out]
                n171 = local write "Remove Offset"(FALSE ("Help")) -> ()
                n172 = Format Into String(format string="Action: Offset Mode >> %s\nAction: Command", Offset_Mode--Enum."Remove" ("Offset Mode")) -> (resulting string=w393:string)  [unwired: 2 in, 1 out]
                n173 = call <vilib>:"Add State(s) to Queue__jki_lib_state_machine.vi"("State(s) in Front (\"\")"=w393, "State(s) in (\"\")"=w399) -> ("States Out"=w398:string)  [unwired: 13 in]
              }
              event "Measure Offset": Value Change {
                # "Measure Offset Value Change Event (Button Pressed)\n()"
                n174 = event-data() -> ()  [unwired: 1 in, 6 out]
                n175 = local write "Measure Offset"(FALSE ("Help")) -> ()
                n176 = Format Into String(format string="Action: Offset Mode >> %s\nAction: Command", Offset_Mode--Enum."Measure" ("Offset Mode")) -> (resulting string=w401:string)  [unwired: 2 in, 1 out]
                n177 = call <vilib>:"Add State(s) to Queue__jki_lib_state_machine.vi"("State(s) in Front (\"\")"=w401, "State(s) in (\"\")"=w407) -> ("States Out"=w406:string)  [unwired: 13 in]
              }
              event "Get Calibration": Value Change {
                # "Get Calibration Value Change Event (Button Pressed)\n()"
                n178 = event-data() -> ()  [unwired: 1 in, 6 out]
                n179 = local write "Get Calibration"(FALSE ("Help")) -> ()
                n180 = Format Into String(format string="Action: Calibrate >> %s\nAction: Command", PrivateEvents--DAQ.setCalibration."Check" ("setCalibration")) -> (resulting string=w409:string)  [unwired: 2 in, 1 out]
                n181 = call <vilib>:"Add State(s) to Queue__jki_lib_state_machine.vi"("State(s) in Front (\"\")"=w409, "State(s) in (\"\")"=w415) -> ("States Out"=w414:string)  [unwired: 13 in]
              }
              event "Self Calibrate": Value Change {
                # "Get Calibration Value Change Event (Button Pressed)\n()"
                n182 = event-data() -> ()  [unwired: 1 in, 6 out]
                n183 = local write "Self Calibrate"(FALSE ("Help")) -> ()
                n184 = Format Into String(format string="Action: Calibrate >> %s\nAction: Command", PrivateEvents--DAQ.setCalibration."Calibrate" ("setCalibration")) -> (resulting string=w416:string)  [unwired: 2 in, 1 out]
                n185 = call <vilib>:"Add State(s) to Queue__jki_lib_state_machine.vi"("State(s) in Front (\"\")"=w416, "State(s) in (\"\")"=w423) -> ("States Out"=w422:string)  [unwired: 13 in]
              }
              event "Show DAQ UI": Value Change {
                # "Get Calibration Value Change Event (Button Pressed)\n()"
                n186 = event-data() -> ()  [unwired: 1 in, 6 out]
                n187 = Format Into String(format string="Action: show DAQ UI >> %s\nAction: Command", "Show DAQ UI") -> (resulting string=w424:string)  [unwired: 2 in, 1 out]
                n188 = call <vilib>:"Add State(s) to Queue__jki_lib_state_machine.vi"("State(s) in Front (\"\")"=w424, "State(s) in (\"\")"=w430) -> ("States Out"=w429:string)  [unwired: 13 in]
              }
              event "Logging": Value Change {
                # "Get Calibration Value Change Event (Button Pressed)\n()"
                n189 = event-data() -> ("NewVal"=w431:bool)  [unwired: 1 in, 5 out]
                n190 = Format Into String(format string="Action: Logging >> %s\nAction: Command", w431) -> (resulting string=w432:string)  [unwired: 2 in, 1 out]
                n191 = call <vilib>:"Add State(s) to Queue__jki_lib_state_machine.vi"("State(s) in Front (\"\")"=w432, "State(s) in (\"\")"=w437) -> ("States Out"=w436:string)  [unwired: 13 in]
              }
              event "....................Graph and UI....................": Value Change {
                # "Do not put any code in this frame.\n(it is a separator no-op)"
                n192 = event-data() -> ()  [unwired: 1 in, 6 out]
                n193 = call <vilib>:"Add State(s) to Queue__jki_lib_state_machine.vi"("State(s) in (\"\")"=w441) -> ("States Out"=w440:string)  [unwired: 14 in]
              }
              event Value Change {
                # "Display Value Change Event (Button Pressed)\n()"
                n194 = event-data() -> ()  [unwired: 1 in, 6 out]
                n195 = call <vilib>:"Add State(s) to Queue__jki_lib_state_machine.vi"("State(s) in Front (\"\")"="UI: Defer Panel Updates >> TRUE\nUI: Update Lockin Graph Labels\nUI: Defer Panel Updates >> FALSE", "State(s) in (\"\")"=w446) -> ("States Out"=w445:string)  [unwired: 13 in]
              }
              event "PS Display": Value Change {
                w449 = "UI: Defer Panel Updates >> TRUE\nUI: Update PS Graph Labels\nUI: Update PS Graph Legend\nUI: Defer Panel Updates >> FALSE"  # UI: Defer Panel Updates >> TRUE UI: Update PS Graph Labels UI: Update PS Graph Legend UI: Defer Panel Updates >> FALSE
                # "Display Value Change Event (Button Pressed)\n()"
                n196 = event-data() -> ()  [unwired: 1 in, 6 out]
                n197 = call <vilib>:"Add State(s) to Queue__jki_lib_state_machine.vi"("State(s) in Front (\"\")"=w449, "State(s) in (\"\")"=w451) -> ("States Out"=w450:string)  [unwired: 13 in]
              }
              event "AI Graph": Plot Attribute Change {
                # "Display Value Change Event (Button Pressed)\n()"
                n198 = event-data() -> ()  [unwired: 1 in, 8 out]
                n199 = call <vilib>:"Add State(s) to Queue__jki_lib_state_machine.vi"("State(s) in Front (\"\")"="UI: Defer Panel Updates >> TRUE\nUI: Sync AI Plot Visibility\nUI: Defer Panel Updates >> FALSE", "State(s) in (\"\")"=w456) -> ("States Out"=w455:string)  [unwired: 13 in]
              }
              event "AO Graph": Value Change {
                # "Display Value Change Event (Button Pressed)\n()"
                n200 = event-data() -> ()  [unwired: 1 in, 6 out]
                n201 = call <vilib>:"Add State(s) to Queue__jki_lib_state_machine.vi"("State(s) in Front (\"\")"="UI: Defer Panel Updates >> TRUE\nUI: Sync AO Plot Visibility\nUI: Defer Panel Updates >> FALSE", "State(s) in (\"\")"=w461) -> ("States Out"=w460:string)  [unwired: 13 in]
              }
              event "Lockin 1": Plot Attribute Change {
                # "Display Value Change Event (Button Pressed)\n()"
                n202 = event-data() -> ()  [unwired: 1 in, 8 out]
                n203 = call <vilib>:"Add State(s) to Queue__jki_lib_state_machine.vi"("State(s) in Front (\"\")"="UI: Defer Panel Updates >> TRUE\nUI: Sync Lockin Plot Visibility\nUI: Defer Panel Updates >> FALSE", "State(s) in (\"\")"=w466) -> ("States Out"=w465:string)  [unwired: 13 in]
              }
              event "Lockin 1", "Lockin 2": Shortcut Menu Selection? (App) {
                # "Display Value Change Event (Button Pressed)\n()"
                n204 = event-data() -> ("ItemTag"=w469:string)  [unwired: 1 in]
                n205 = Equal?(x="APP_SC_CLEAR_GRAPH", y=w469) -> (x = y?=w467:bool)
                n206 = Bundle By Name(cluster=w470, "clear lockin charts"=w467) -> (w471:T65)
                n207 = event-data("Discard?"=w467) -> ()  [unwired: 1 in, 1 out]
                n208 = call <vilib>:"Add State(s) to Queue__jki_lib_state_machine.vi"("State(s) in Front (\"\")"="", "State(s) in (\"\")"=w475) -> ("States Out"=w474:string)  [unwired: 13 in]
              }
              event "Disable All", "Enable All": Value Change {
                # "AI Disable or Enable Change Event (Button Pressed)\n()"
                n209 = event-data() -> ("CtlRef"=w476:refnum<vi>)  [unwired: 1 in, 5 out]
                n210 = control-ref of="Disable All"() -> (w478:refnum<vi>)
                n211 = Equal?(x=w476, y=w478) -> (x = y?=w477:bool)
                n212 = flat-sequence {
                  tunnel: w477 -> [_]
                  frame #0 {
                    n213 = local write "Enable All"(FALSE ("Disable all AI Ref")) -> ()
                    n214 = local write "Disable All"(FALSE ("Disable all AI Ref")) -> ()
                  }
                }
                n215 = Select(t="Disable" ("Arguments (\"\")"), s=w477, f="ALL 1" ("Arguments (\"\")")) -> (s? t:f=w479:string)
                n216 = call <vilib>:"Build State String with Arguments__JKI_lib_State_Machine.vi"("Arguments (\"\")"=w479, "State"="UI: Update AI REF Channels") -> ("State with Arguments"=w484:string)  [unwired: 4 in]
                n217 = call <vilib>:"Add State(s) to Queue__jki_lib_state_machine.vi"("State(s) in Front (\"\")"=w484, "State(s) at Back (\"\")"="Action: AI Channels\nAction: Command") -> ("States Out"=w482:string)  [unwired: 13 in]
                n218 = call <vilib>:"Add State(s) to Queue__jki_lib_state_machine.vi"("State(s) in Front (\"\")"=w482, "State(s) in (\"\")"=w489) -> ("States Out"=w488:string)  [unwired: 13 in]
              }
              event "AI Graph All", "AI Graph None": Value Change {
                # "AI Graph All/None Value Change Event (Button Pressed)\n()"
                n219 = event-data() -> ("CtlRef"=w499:refnum<vi>)  [unwired: 1 in, 5 out]
                n220 = control-ref of="AI Graph All"() -> (w498:refnum<vi>)
                n221 = Equal?(x=w499, y=w498) -> (x = y?=w495:bool)
                n222 = Select(t="ALL" ("Arguments (\"\")"), s=w495, f="NONE" ("Arguments (\"\")")) -> (s? t:f=w493:string)
                n223 = Format Into String(format string="UI: Defer Panel Updates >> TRUE\nUI: AI Graphs Plot Visibility >> %s\nUI: Defer Panel Updates >> FALSE", w493) -> (resulting string=w492:string)  [unwired: 2 in, 1 out]
                n224 = call <vilib>:"Add State(s) to Queue__jki_lib_state_machine.vi"("State(s) in Front (\"\")"=w492, "State(s) in (\"\")"=w503) -> ("States Out"=w502:string)  [unwired: 13 in]
              }
              event "AO Graph All", "AO Graph None": Value Change {
                # "AO Graph All Value Change Event (Button Pressed)\n()"
                n225 = event-data() -> ("CtlRef"=w511:refnum<vi>)  [unwired: 1 in]
                n226 = control-ref of="AO Graph All"() -> (w510:refnum<vi>)
                n227 = Equal?(x=w511, y=w510) -> (x = y?=w509:bool)
                n228 = Select(t="ALL" ("Arguments (\"\")"), s=w509, f="NONE" ("Arguments (\"\")")) -> (s? t:f=w505:string)
                n229 = Format Into String(format string="UI: Defer Panel Updates >> TRUE\nUI: AO Graphs Plot Visibility >> %s\nUI: Defer Panel Updates >> FALSE", w505) -> (resulting string=w504:string)  [unwired: 2 in, 1 out]
                n230 = call <vilib>:"Add State(s) to Queue__jki_lib_state_machine.vi"("State(s) in Front (\"\")"=w504, "State(s) in (\"\")"=w515) -> ("States Out"=w514:string)  [unwired: 13 in]
              }
              event "REF Graph All", "REF Graph None": Value Change {
                # "AO Graph All Value Change Event (Button Pressed)\n()"
                n231 = event-data() -> ("CtlRef"=w523:refnum<vi>)  [unwired: 1 in]
                n232 = control-ref of="REF Graph All"() -> (w522:refnum<vi>)
                n233 = Equal?(x=w523, y=w522) -> (x = y?=w521:bool)
                n234 = Select(t="ALL" ("Arguments (\"\")"), s=w521, f="NONE" ("Arguments (\"\")")) -> (s? t:f=w517:string)
                n235 = Format Into String(format string="UI: Defer Panel Updates >> TRUE\nUI: REF Graphs Plot Visibility >> %s\nUI: Defer Panel Updates >> FALSE", w517) -> (resulting string=w516:string)  [unwired: 2 in, 1 out]
                n236 = call <vilib>:"Add State(s) to Queue__jki_lib_state_machine.vi"("State(s) in Front (\"\")"=w516, "State(s) in (\"\")"=w527) -> ("States Out"=w526:string)  [unwired: 13 in]
              }
              event "Lockin Graph All", "Lockin Graph None", "Lockin Graph All 2", "Lockin Graph None 2": Value Change {
                # "Lockin Graph All Value Change Event (Button Pressed)\n()"
                n237 = event-data() -> ("CtlRef"=w531:refnum<vi>)  [unwired: 1 in]
                n238 = control-ref of="Lockin Graph All"() -> (w538:refnum<vi>)
                n239 = control-ref of="Lockin Graph All 2"() -> (w532:refnum<vi>)
                n240 = Equal?(x=w531, y=w538) -> (x = y?=w529:bool)
                n241 = Equal?(x=w531, y=w532) -> (x = y?=w530:bool)
                n242 = Or(x=w529, y=w530) -> (x .or. y?=w528:bool)
                n243 = Select(t="ALL" ("Arguments (\"\")"), s=w528, f="NONE" ("Arguments (\"\")")) -> (s? t:f=w534:string)
                n244 = Format Into String(format string="UI: Defer Panel Updates >> TRUE\nUI: Lockin Graphs Plot Visibility >> %s\nUI: Defer Panel Updates >> FALSE", w534) -> (resulting string=w533:string)  [unwired: 2 in, 1 out]
                n245 = call <vilib>:"Add State(s) to Queue__jki_lib_state_machine.vi"("State(s) in Front (\"\")"=w533, "State(s) in (\"\")"=w542) -> ("States Out"=w541:string)  [unwired: 13 in]
              }
              event "X/R Range", "Y/Theta Range", "XY Range": Value Change {
                # "X/R Range, Y/Theta Range, XY Range Value Change Event\n(this executes UI: Update Lockin Graph Range)"
                n246 = event-data() -> ()  [unwired: 1 in, 6 out]
                n247 = call <vilib>:"Add State(s) to Queue__jki_lib_state_machine.vi"("State(s) in Front (\"\")"="UI: Defer Panel Updates >> TRUE\nUI: Update Lockin Graph Range\nUI: Defer Panel Updates >> FALSE", "State(s) in (\"\")"=w547) -> ("States Out"=w546:string)  [unwired: 13 in]
              }
              event "Output": Value Change {
                # "Y Axis (Output) Value Change Event\n(this executes UI: Show Hide AO Waveform Graphs)"
                n248 = event-data() -> ()  [unwired: 1 in, 6 out]
                n249 = call <vilib>:"Add State(s) to Queue__jki_lib_state_machine.vi"("State(s) in Front (\"\")"="UI: Defer Panel Updates >> TRUE\nUI: Show Hide AO Waveform Graphs\nUI: Defer Panel Updates >> FALSE", "State(s) in (\"\")"=w552) -> ("States Out"=w551:string)  [unwired: 13 in]
              }
              event "X Scale": Value Change {
                # "X Axis Value Change Event\n(this executes UI: Update Waveform Graph Labels)"
                n250 = event-data() -> ()  [unwired: 1 in, 6 out]
                n251 = call <vilib>:"Add State(s) to Queue__jki_lib_state_machine.vi"("State(s) in Front (\"\")"="UI: Defer Panel Updates >> TRUE\nUI: Update Waveform Graph Labels\nUI: Defer Panel Updates >> FALSE", "State(s) in (\"\")"=w557) -> ("States Out"=w556:string)  [unwired: 13 in]
              }
              event "export mode": Value Change {
                # "PS export mode Value Change Event\n(this executes UI: Update PS Graph Labels)"
                n252 = event-data() -> ()  [unwired: 1 in, 6 out]
                n253 = call <vilib>:"Add State(s) to Queue__jki_lib_state_machine.vi"("State(s) in Front (\"\")"="UI: Defer Panel Updates >> TRUE\nUI: Update PS Graph Labels\nUI: Defer Panel Updates >> FALSE", "State(s) in (\"\")"=w562) -> ("States Out"=w561:string)  [unwired: 13 in]
              }
              event "....................Dynamic Events....................": Value Change {
                # "Do not put any code in this frame.\n(it is a separator no-op)"
                n254 = event-data() -> ()  [unwired: 1 in, 6 out]
                n255 = call <vilib>:"Add State(s) to Queue__jki_lib_state_machine.vi"("State(s) in (\"\")"=w566) -> ("States Out"=w565:string)  [unwired: 14 in]
              }
              event User Event {
                # "<SMO Protected Events.StopProcesses>: User Event"
                n256 = event-data() -> ()  [unwired: 1 in, 5 out]
                n257 = call <vilib>:"Add State(s) to Queue__jki_lib_state_machine.vi"("State(s) in Front (\"\")"="Macro: Exit", "State(s) in (\"\")"=w571) -> ("States Out"=w570:string)  [unwired: 13 in]
              }
              event User Event {
                # "<SMO Protected Events.AbortProcesses>: User Event"
                # "On Abort, no nice macro exit, but exit right away"
                n258 = event-data() -> ()  [unwired: 1 in, 5 out]
                n259 = call <vilib>:"Add State(s) to Queue__jki_lib_state_machine.vi"("State(s) in Front (\"\")"="Exit", "State(s) in (\"\")"=w576) -> ("States Out"=w575:string)  [unwired: 13 in]
              }
              event User Event {
                # "<SMO.UI Public Events.UI Hidden>: User Event"
                n260 = event-data() -> ()  [unwired: 1 in, 5 out]
                n261 = call <vilib>:"Add State(s) to Queue__jki_lib_state_machine.vi"("State(s) in (\"\")"=w580) -> ("States Out"=w579:string)  [unwired: 14 in]
              }
              event User Event {
                # "<DAQ SMO Public Events.Error>: User Event"
                n262 = event-data() -> ()  [unwired: 1 in, 7 out]
                n263 = call <vilib>:"Add State(s) to Queue__jki_lib_state_machine.vi"("State(s) in (\"\")"=w584) -> ("States Out"=w583:string)  [unwired: 14 in]
              }
              event User Event {
                # "<DAQ SMO Public Events.State>: User Event"
                n264 = event-data() -> ("SMO State"=w585:T67)  [unwired: 1 in, 4 out]
                n265 = case shown="\"Started\"" w585 {
                  tunnel: ["UI: Enable Buttons" ("State Queue") "//DONE: Stop\n//DONE: Start" ("State Queue")] -> w586
                  frame "Started" {
                  }
                  frame Default {
                  }
                }
                n266 = call <vilib>:"Add State(s) to Queue__jki_lib_state_machine.vi"("State(s) in Front (\"\")"=w586, "State(s) in (\"\")"=w590) -> ("States Out"=w589:string)  [unwired: 13 in]
              }
              event User Event {
                # "<DAQ Public Events.getDAQState>: User Event"
                n267 = event-data() -> ("status"=w597:T33)  [unwired: 1 in, 4 out]
                n268 = Get Date/Time In Seconds() -> (seconds since 1Jan1904=w600:timestamp)
                n269 = Format Into String(w597) -> (resulting string=→"Inst.DAQ State":string)  [unwired: 3 in, 1 out]
                n270 = To Double Precision Float(number=w600) -> (double precision float=→"State Time":dbl)
                n271 = Bundle By Name(cluster=w598, "DAQ state"=w597) -> (w603:T65)
                n272 = case shown="\"sweeping\"" w597 {
                  frame Default {
                  }
                  frame "sweeping" {
                    n273 = call <userlib>:"MGI Milliseconds Since Last Reset.vi"("Reset (F)"=TRUE) -> ()  [unwired: 5 in, 2 out]
                  }
                }
                n274 = Format Into String(w597) -> (resulting string=w596:string)  [unwired: 3 in, 1 out]
                n275 = call <vilib>:"Build State String with Arguments__JKI_lib_State_Machine.vi"("Arguments (\"\")"=w596, "State"="UI: Update Status") -> ("State with Arguments"=w595:string)  [unwired: 4 in]
                n276 = call <vilib>:"Add State(s) to Queue__jki_lib_state_machine.vi"("State(s) in Front (\"\")"=w595, "State(s) in (\"\")"="UI: Defer Panel Updates >> TRUE\nUI: Update Booleans\nUI: Defer Panel Updates >> FALSE" ("State")) -> ("States Out"=w594:string)  [unwired: 13 in]
                n277 = call <vilib>:"Add State(s) to Queue__jki_lib_state_machine.vi"("State(s) in Front (\"\")"=w594, "State(s) in (\"\")"=w606) -> ("States Out"=w605:string)  [unwired: 13 in]
              }
              event User Event {
                # "== T when \"start\" button pressed"
                # "<DAQ Public Events.getWaveforms>: User Event"
                n278 = event-data() -> ("AO"=w613:waveform(dbl)[], "AI"=w612:waveform(dbl)[], "REF_X"=w611:waveform(dbl)[], "REF_Y"=w610:waveform(dbl)[])  [unwired: 1 in, 4 out]
                n279 = Unbundle By Name(w615) -> ("update waveform graphs"=w618:bool)
                n280 = Bundle By Name(cluster=w615, "update waveform graphs"=FALSE ("update graphs"), "getAll.Waveforms.AO"=w613, "getAll.Waveforms.AI"=w612, "getAll.Waveforms.REF_X"=w611, "getAll.Waveforms.REF_Y"=w610) -> (w614:T65)
                n281 = Select(t="Macro: Initialize Waveform Graphs", s=w618, f="Macro: Update Waveform Graphs") -> (s? t:f=w608:string)
                n282 = call <vilib>:"Add State(s) to Queue__jki_lib_state_machine.vi"("State(s) in Front (\"\")"=w608, "State(s) in (\"\")"=w621) -> ("States Out"=w620:string)  [unwired: 13 in]
              }
              event User Event {
                # "== T when \"start\" button pressed"
                # "<DAQ Public Events.getResults>: User Event"
                n283 = event-data() -> ("Results"=w631:T59)  [unwired: 1 in, 4 out]
                n284 = Unbundle By Name(w627) -> ("update lockin graphs"=w626:bool)
                n285 = Bundle By Name(cluster=w627, "update lockin graphs"=FALSE, "getAll.Results"=w631) -> (w632:T65)
                n286 = Select(t="Macro: Initialize Lockin Graphs", s=w626, f="") -> (s? t:f=w622:string)
                n287 = call <vilib>:"Add State(s) to Queue__jki_lib_state_machine.vi"("State(s) in Front (\"\")"=w622, "State(s) at Back (\"\")"="Macro: Update Lockin Graphs") -> ("States Out"=w625:string)  [unwired: 13 in]
                n288 = call <vilib>:"Add State(s) to Queue__jki_lib_state_machine.vi"("State(s) in Front (\"\")"=w625, "State(s) in (\"\")"=w634) -> ("States Out"=w633:string)  [unwired: 13 in]
              }
              event User Event {
                # "<DAQ Public Events.getCalibration>: User Event"
                n289 = event-data() -> ("Calibration"=w635:T23)  [unwired: 1 in, 4 out]
                "Cal Info" <- w635
                n290 = Bundle By Name(cluster=w636, "UI Config.DAQ.Calibration"=w635) -> (w637:T65)
                n291 = call <vilib>:"Add State(s) to Queue__jki_lib_state_machine.vi"("State(s) in Front (\"\")"="", "State(s) in (\"\")"=w641) -> ("States Out"=w640:string)  [unwired: 13 in]
              }
              event User Event {
                # "<DAQ Public Events.getAOChannels>: User Event"
                n292 = event-data() -> ("Channels: AO"=w643:T6)  [unwired: 1 in, 4 out]
                n293 = local write "AO Channels"(w643) -> ()
                n294 = Bundle By Name(cluster=w644, "UI Config.Channels.Cfg_AO"=w643) -> (w645:T65)
                n295 = call <vilib>:"Add State(s) to Queue__jki_lib_state_machine.vi"("State(s) in Front (\"\")"="" ("f"), "State(s) in (\"\")"=w648) -> ("States Out"=w647:string)  [unwired: 13 in]
              }
              event User Event {
                # "<DAQ Public Events.getAIChannels>: User Event"
                n296 = event-data() -> ("Channels.AI"=w651:T4)  [unwired: 1 in, 4 out]
                n297 = Bundle By Name(cluster=w650, "UI Config.Channels.Cfg_AI"=w651) -> (w652:T65)
                n298 = local write "AI Channels"(w651) -> ()
                n299 = call <vilib>:"Add State(s) to Queue__jki_lib_state_machine.vi"("State(s) in Front (\"\")"="" ("State(s) in Front (\"\")"), "State(s) in (\"\")"=w655) -> ("States Out"=w654:string)  [unwired: 13 in]
              }
              event User Event {
                # "<DAQ Public Events.getREFChannels>: User Event"
                n300 = event-data() -> ("Channels: REF"=w657:T2)  [unwired: 1 in, 4 out]
                n301 = Bundle By Name(cluster=w658, "UI Config.Channels.Cfg_REF"=w657) -> (w659:T65)
                n302 = local write "REF Channels"(w657) -> ()
                n303 = call <vilib>:"Add State(s) to Queue__jki_lib_state_machine.vi"("State(s) in Front (\"\")"="UI: Defer Panel Updates >> TRUE\nUI: Update Channel Ring\nUI: Update AI REF Channel Ring\nUI: Remove Unused References\nUI: Defer Panel Updates >> FALSE", "State(s) in (\"\")"=w662) -> ("States Out"=w661:string)  [unwired: 13 in]
              }
              event User Event {
                # "<DAQ Public Events.getSweepChannels>: User Event"
                n304 = event-data() -> ("Channels.Sweep"=w663:T55)  [unwired: 1 in, 4 out]
                n305 = Bundle By Name(cluster=w664, "UI Config.Sweep"=w663) -> (w665:T65)
                n306 = call <vilib>:"Add State(s) to Queue__jki_lib_state_machine.vi"("State(s) in Front (\"\")"="UI: Update Sweep Config", "State(s) in (\"\")"=w669) -> ("States Out"=w668:string)  [unwired: 13 in]
              }
              event User Event {
                # "<DAQ Public Events.getSweepWaveforms>: User Event"
                n307 = event-data() -> ("AO"=w682:waveform(dbl)[], "AI"=w681:waveform(dbl)[], "X"=w680:waveform(dbl)[], "Y"=w679:waveform(dbl)[])  [unwired: 1 in, 4 out]
                n308 = Bundle By Name(cluster=w678, "getAll.SweepWaveforms.AO"=w682, "getAll.SweepWaveforms.AI"=w681, "getAll.SweepWaveforms.X"=w680, "getAll.SweepWaveforms.Y"=w679) -> (w683:T65)
                n309 = Unbundle By Name(w678) -> ("DAQ state"=w670:T33)
                n310 = Get Date/Time In Seconds() -> (seconds since 1Jan1904=w672:timestamp)
                n311 = To Double Precision Float(number=w672) -> (double precision float=→"Sweep Time":dbl)
                n312 = Equal?(x=Status--enum."idle" ("getAll.DAQ state"), y=w670) -> (x = y?=w675:bool)
                n313 = Format Into String(w670) -> ()  [unwired: 3 in, 2 out]
                n314 = Select(t="Macro: Initialize Waveform Graphs", s=w675, f="UI: Update Sweep Graphs") -> (s? t:f=w673:string)
                n315 = call <vilib>:"Add State(s) to Queue__jki_lib_state_machine.vi"("State(s) in Front (\"\")"=w673, "State(s) in (\"\")"=w686) -> ("States Out"=w685:string)  [unwired: 13 in]
              }
              event User Event {
                # "<DAQ Public Events.getDAQconfig>: User Event"
                n316 = event-data() -> ("New Ch []"=w687:T9)  [unwired: 1 in]
                n317 = Bundle By Name(cluster=w688, "UI Config.DAQ.Configuration"=w687) -> (w689:T65)
                n318 = local write "DAQ Config"(w687) -> ()
                n319 = call <vilib>:"Add State(s) to Queue__jki_lib_state_machine.vi"("State(s) in Front (\"\")"="UI: Defer Panel Updates >> TRUE\nUI: Update AI Waveform Graphs Legends\nUI: Update AI Waveform Graphs Colors\nUI: Update AO Waveform Graphs Legends\nUI: Update AO Waveform Graphs Colors\nUI: Defer Panel Updates >> FALSE", "State(s) in (\"\")"=w693) -> ("States Out"=w692:string)  [unwired: 13 in]
              }
              event User Event {
                # "<DAQ Public Events.getSampling>: User Event"
                n320 = event-data() -> ("Sampling"=w696:T48)  [unwired: 1 in]
                n321 = Unbundle By Name(w696) -> ("Sampling.Fs"=→"Fs (S/s)":dbl, "Sampling.#s"=→"#s (S)":i32)
                n322 = Bundle By Name(cluster=w697, "UI Config.DAQ.cfg.Sampling"=w696) -> (w698:T65)
                n323 = call <vilib>:"Add State(s) to Queue__jki_lib_state_machine.vi"("State(s) in Front (\"\")"="", "State(s) in (\"\")"=w702) -> ("States Out"=w701:string)  [unwired: 13 in]
              }
              event User Event {
                # "<DAQ Public Events.getInputGain>: User Event"
                n324 = event-data() -> ("Input Gain"=w703:T17)  [unwired: 1 in, 4 out]
                n325 = Bundle By Name(cluster=w704, "UI Config.Amplifers.Gain_AI"=w703) -> (w705:T65)
                n326 = local write "Input Gain"(w703) -> ()
                n327 = call <vilib>:"Add State(s) to Queue__jki_lib_state_machine.vi"("State(s) in Front (\"\")"="", "State(s) in (\"\")"=w709) -> ("States Out"=w708:string)  [unwired: 13 in]
              }
              event User Event {
                # "<DAQ Public Events.getOutputGain>: User Event"
                n328 = event-data() -> ("Output Gain"=w710:T17)  [unwired: 1 in, 4 out]
                n329 = Bundle By Name(cluster=w711, "UI Config.Amplifers.Gain_AO"=w710) -> (w712:T65)
                n330 = local write "Output Gain"(w710) -> ()
                n331 = call <vilib>:"Add State(s) to Queue__jki_lib_state_machine.vi"("State(s) in Front (\"\")"="", "State(s) in (\"\")"=w716) -> ("States Out"=w715:string)  [unwired: 13 in]
              }
              event User Event {
                # "<DAQ Public Events.getInputOffset>: User Event"
                n332 = event-data() -> ("Input Offset"=w717:T17)  [unwired: 1 in, 4 out]
                n333 = Bundle By Name(cluster=w718, "UI Config.Amplifers.Offset_AI"=w717) -> (w719:T65)
                n334 = local write "Input Offsets"(w717) -> ()
                n335 = call <vilib>:"Add State(s) to Queue__jki_lib_state_machine.vi"("State(s) in Front (\"\")"="", "State(s) in (\"\")"=w723) -> ("States Out"=w722:string)  [unwired: 13 in]
              }
            }
          }
          frame "---------- Core ----------" {
            # "Do not put any code in this frame.\n(it is a separator no-op)"
            n336 = call <vilib>:"Add State(s) to Queue__jki_lib_state_machine.vi"("State(s) in (\"\")"=w728) -> ("States Out"=w727:string)  [unwired: 14 in]
          }
          frame Default {
            w739 = 42 items=["No error", "Argument error", "Memory is full", "Out of zone", "End of file", "File already open", "Generic file I/O error", "File not found", "File permission error", "Disk is full", "Duplicate path", "Too many files open", "System feature not enabled", "Resource file not found", "Cannot add resource", "Resource not found", "Image not found", "Image memory error", "Pen does not exist", "Config type invalid", "Config token not found", "Config parse error", "Config memory error", "Bad external code format", "Bad external code offset", "External code not present", "Null window", "Destroy window error", "Null menu", "Print aborted", "Bad print record", "Print driver error", "Windows error during printing", "Memory error during printing", "Print dialog error", "Generic print error", "Invalid device refnum", "Device not found", "Device parameter error", "Device unit error", "Cannot open device", "Device call aborted", "Generic error", "Cancelled by user", "Object ID too low", "Object ID too high", "Object not in heap", "Unknown heap", "Unknown object (invalid DefProc)", "Unknown object (DefProc not in table)", "Message out of range", "Invalid (null) method", "Unknown message", "Manager call not supported", "Bad address", "Network operation in progress", "Network operation timed out", "Connection is busy", "Network attribute not supported", "Network error", "Address in use", "System out of memory", "Connection aborted", "Connection refused", "Not connected", "Already connected", "Connection closed", "Initialization error (interapplication manager)", "Bad occurrence", "Wait on unbound occurrence handler", "Occurrence queue overflow", "Datalog type conflict", "Unused", "Unrecognized type (interapplication manager)", "Memory corrupt", "Failed to make temporary DLL", "Old CIN version", "Drag socket not found", "Failed to load drop-object", "Failed to register OLE object", "Failed to release OLE object", "Format specifier type mismatch", "Unknown format specifier", "Too few format specifiers", "Too many format specifiers", "Scan failed", "Newer CIN version", "Error converting to variant", "Runtime menu error", "Password tampered", "Variant attribute not found", "Incompatible variant data type", "Event data is not available", "Event Store is not present", "Occurrence is not found", "Event Queue is not created", "Event info is not available", "Refnum passed is NULL", "Error retrieving Class GUID", "Error retrieving CoClass GUID", "Error retrieving TypeLib GUID.", "Bad built application magic bytes.", "Specific driver is different from the specific driver associated with the Logical Name.", "There is no session opened to the class driver.", "Max Error", "MAX - Error with config objects", "MAX - Error loading configuration", "MAX - Group not supported"]
            # "Current State"
            # "Do not delete, rename, or modify this frame.\n(this is used to capture unhandled states and typos)"
            # "Handle mistyped state name (developer tool)"
            n337 = Format Into String(format string="Software Exception: Unhandled State \"%s\"." ("message"), error in=w735, w730) -> (resulting string=w738:string, error out=w737:errorcluster)  [unwired: 1 in]
            n338 = call <vilib>:"Error Cluster From Error Code.vi"("show call chain? (False)"=TRUE, "error in (no error)"=w737, "error message (\"\")"=w738, "error code (0)"=w739) -> ("error out"=w736:errorcluster)  [unwired: 5 in]
            n339 = call <vilib>:"Add State(s) to Queue__jki_lib_state_machine.vi"("State(s) in (\"\")"=w734) -> ("States Out"=w733:string)  [unwired: 14 in]
          }
          frame "Initialize Core Data" {
            # "Do not delete, rename, or modify this frame.\n(this is used to determine panel behavior on exit)"
            # "originally closed?"
            # "exe?"
            # "If panel starts closed or is an EXE, then close it when we exit"
            n340 = property class="VI"() -> ("Front Panel.Open"=w749:bool)  [unwired: 2 in, 2 out]
            n341 = property class="App"() -> ("App.Kind"=w748:T34)  [unwired: 2 in, 2 out]
            n342 = control-ref of="Current VI Reference"() -> (w742:refnum<vi>)
            n343 = Not(x=w749) -> (.not. x?=w746:bool)
            n344 = Equal?(x=w748, y=T34."Run Time System" ("Application:Kind")) -> (x = y?=w745:bool)
            n345 = Or(x=w746, y=w745) -> (x .or. y?=w743:bool)
            n346 = Bundle By Name(cluster=w744, "Core.Current VI Reference"=w742, "Core.Close Panel on Exit?"=w743) -> (w751:T65)
            n347 = call <vilib>:"Add State(s) to Queue__jki_lib_state_machine.vi"("State(s) in (\"\")"=w753) -> ("States Out"=w752:string)  [unwired: 14 in]
          }
          frame "Error Handler" {
            w761 = errorcluster {"status"=FALSE, "code"=0, "source"=""}  # No error
            # "There was an error while handling the error.\nStop the process. This error can only occur if public events references are invalid or if the state machine object is destroyed."
            # "Overwrite this method to handle errors and pass to parent if not handled. Parent will fire a public event if the error is not handled up the chain of classes."
            # "Handle any errors here.\nYou can also output any states to clean-up after errors occur"
            n348 = Unbundle By Name(w759) -> ("SelfRef"=w765:refnum<class "Instrument UI.Lockin.lvclass">)
            n349 = call-dynamic "Handle Error.vi"("Stop on Unhandled Error (T)"=FALSE, "error in"=w764, "SMO"=w765) -> ("handling error"=w762:errorcluster, "Unhandled error"=w760:errorcluster)  [unwired: 6 in, 1 out]
            n350 = Bundle By Name(cluster=w759, "Core.Last Error.remaining states"=w756, "Core.Last Error.error"=w760) -> (w758:T65)
            n351 = Select(t="Exit", s=w762, f="Macro: Post Error Handling") -> (s? t:f=w755:string)
          }
          frame "Exit" {
            # "Do not put any code in this frame.\n(No errors that occur here will be handled.)"
            n352 = Unbundle By Name(w768) -> ("Core.Last Error.error"=w767:errorcluster)
            n353 = call <vilib>:"Add State(s) to Queue__jki_lib_state_machine.vi"("State(s) in (\"\")"=w772) -> ("States Out"=w771:string)  [unwired: 14 in]
          }
          frame "---------- Data ----------" {
            # "Do not put any code in this frame.\n(It is a separator no-op. You can make a copy of this frame to create a new Data frame)"
            n354 = call <vilib>:"Add State(s) to Queue__jki_lib_state_machine.vi"("State(s) in (\"\")"=w777) -> ("States Out"=w776:string)  [unwired: 14 in]
          }
          frame "Data: Initialize" {
            w778 = FALSE  # clear lockin charts
            w779 = waveform(dbl)[][] []  # Waveform Charts
            w780 = FALSE  # update lockin graphs
            w781 = FALSE  # update waveform graphs
            w785 = T68 {"Current VI Reference"=refnum, "Close Panel on Exit?"=FALSE, "Last Error"={"error"={"status"=FALSE, "code"=0, "source"=""}, "previous state"="", "remaining states"=""}, "Shutdown?"=FALSE}  # Core
            w784 = refnum<vi> refnum  # Front Panel
            w783 = Status--enum."idle"  # DAQ state
            (unwired) string[] []  # Plot Names
            w787 = refnum<class "Instrument.Lockin.lvclass"> refnum  # Lockin
            w793 = T46 {"Channels"={"Cfg_AO"=[], "Cfg_AI"=[], "Cfg_REF"=[]}, "DAQ"={"Configuration"=[], "cfg.Sampling"={"Sampling"={"Fs"=0.0, "#s"=0}, "sample mode"=0, "Fs Mode"=enum."Manual", "Fs Multiplier"=0.0, "Refresh Rate (Hz)"=0.0, "Decimation.PreDSP"=0, "Decimation.PostDSP"=0, "Fs.Output"=0.0}, "Calibration"=[], "Simulation mode"=enum."AI = HW simulated"}, "PreFilter"={"60 Hz"=FALSE, "Low Pass"=FALSE, "Low Pass Cutoff (Hz)"=0.0}, "Amplifers"={"Offset_AI"=[], "Gain_AI"=[], "Gain_AO"=[]}, "Limit Amplitude"={"Limit?"=FALSE, "Limit (V)"=0.0}, "Limit DC"={"Limit?"=FALSE, "Limit (V)"=0.0}, "Link Frequencies"={"Link?"=FALSE, "Frequency (Hz)"=0.0}, "Sweep"={"sweepTime"=0.0, "initialWaitTime"=0.0, "returnToStart"=FALSE, "sweepChannels"=[]}, "Plot"={"visibility.AI"=[], "visibility.AO"=[], "visibility.Lockin"=[], "Display 1"=enum."X", "Display 2"=enum."X"}, "Function Option"={"Option?"=FALSE, "Duty Cycle (%)"=0.0}}  # UI Config
            w794 = cluster{"Command":variant, "Data":variant} {"Command"=variant, "Data"=variant}  # Message
            w782 = T57 {"DAQ State"=enum."idle", "Waveforms"={"AO"=[], "AI"=[], "REF_X"=[], "REF_Y"=[], "X"=[], "Y"=[]}, "Results"={"Time Stamp"=timestamp(0 s since 1904-01-01), "Results (Dictionary)"=[]}, "SweepWaveforms"={"AO"=[], "AI"=[], "X"=[], "Y"=[]}}  # getAll
            w795 = refnum<class "Configuration.lvclass"> refnum  # Configuration
            w796 = T61 {"Booleans"={"Start"=refnum, "Pause"=refnum, "Reset"=refnum, "Trigger"=refnum, "Help"=refnum, "Close"=refnum, "Start Sweep"=refnum, "Stop Sweep"=refnum}, "Clusters"={"AO Channels"=refnum, "AI Channels"=refnum, "REF Channels"=refnum, "DAQ Config"=refnum, "Sweep Channels"=refnum, "Cal Info"=refnum}, "Graphs"={"AI Graph"=refnum, "AO Graph"=refnum, "REF Graph"=refnum, "Lockin 1"=refnum, "Lockin 2"=refnum, "Lockin XY"=refnum, "Sweep X Graph"=refnum, "Sweep Y Graph"=refnum, "Sweep AI Graph"=refnum, "Sweep AO Graph"=refnum, "PS WFGraph"=refnum, "PS Chart"=refnum}}  # References
            # "do not delete - used by framework"
            # "Initialize the shift-register data, here.\n(data names are defined by what you wire into the bundle function)"
            n355 = call <userlib>:"Read Instrument.vi"("error in (no error)"=w789, "Instrument UI in"=w791) -> ("error out"=w788:errorcluster, "Instrument"=w792:refnum<class "Instrument.lvclass">)  [unwired: 7 in, 1 out]
            n356 = To More Specific Class(target class=w787, reference=w792, error in=w788) -> (specific class reference=w786:refnum<class "Instrument.Lockin.lvclass">, error out=w790:errorcluster)
            n357 = Bundle("Core"=w785, "SelfRef"=w791, "Lockin"=w786, "Configuration"=w795, "UI Config"=w793, "DAQ state"=w783, "getAll"=w782, "Waveform Charts"=w779, "References"=w796, "Message"=w794, "Front Panel"=w784, "update waveform graphs"=w781, "update lockin graphs"=w780, "clear lockin charts"=w778) -> (w798:T65)  [unwired: 1 in]
            n358 = call <vilib>:"Add State(s) to Queue__jki_lib_state_machine.vi"("State(s) in (\"\")"=w800) -> ("States Out"=w799:string)  [unwired: 14 in]
          }
          frame "Data: Initialize Control References" {
            n359 = Unbundle By Name(w802) -> ("Core.Current VI Reference"=w801:refnum<vi>)
            n360 = control-ref of="Start"() -> (w810:refnum<vi>)
            n361 = control-ref of="Pause"() -> (w809:refnum<vi>)
            n362 = control-ref of="Reset"() -> (w808:refnum<vi>)
            n363 = control-ref of="Help"() -> (w807:refnum<vi>)
            n364 = control-ref of="Close"() -> (w806:refnum<vi>)
            n365 = control-ref of="Start Sweep"() -> (w805:refnum<vi>)
            n366 = control-ref of="Stop Sweep"() -> (w804:refnum<vi>)
            n367 = control-ref of="AO Channels"() -> (w816:refnum<vi>)
            n368 = control-ref of="AI Channels"() -> (w811:refnum<vi>)
            n369 = control-ref of="REF Channels"() -> (w815:refnum<vi>)
            n370 = control-ref of="DAQ Config"() -> (w814:refnum<vi>)
            n371 = control-ref of="Sweep Channels"() -> (w813:refnum<vi>)
            n372 = control-ref of="Cal Info"() -> (w812:refnum<vi>)
            n373 = property class="VI"(reference=w801) -> ("Front Panel"=w803:refnum<vi>)  [unwired: 1 in, 2 out]
            n374 = Bundle By Name(cluster=w802, "References.Booleans.Start"=w810, "References.Booleans.Pause"=w809, "References.Booleans.Reset"=w808, "References.Booleans.Help"=w807, "References.Booleans.Close"=w806, "References.Booleans.Start Sweep"=w805, "References.Booleans.Stop Sweep"=w804, "References.Clusters.AO Channels"=w816, "References.Clusters.AI Channels"=w811, "References.Clusters.REF Channels"=w815, "References.Clusters.DAQ Config"=w814, "References.Clusters.Sweep Channels"=w813, "References.Clusters.Cal Info"=w812, "Front Panel"=w803) -> (w817:T65)
            n375 = call <vilib>:"Add State(s) to Queue__jki_lib_state_machine.vi"("State(s) in (\"\")"=w821) -> ("States Out"=w820:string)  [unwired: 14 in]
          }
          frame "Data: Initialize Graph References" {
            n376 = control-ref of="REF Graph"() -> (w822:refnum<vi>)
            n377 = control-ref of="Lockin 1"() -> (w832:refnum<vi>)
            n378 = control-ref of="Lockin 2"() -> (w831:refnum<vi>)
            n379 = control-ref of="AI Graph"() -> (w834:refnum<vi>)
            n380 = control-ref of="AO Graph"() -> (w833:refnum<vi>)
            n381 = control-ref of="Lockin XY"() -> (w830:refnum<vi>)
            n382 = control-ref of="Sweep X"() -> (w823:refnum<vi>)
            n383 = control-ref of="Sweep Y"() -> (w824:refnum<vi>)
            n384 = control-ref of="Sweep AI"() -> (w825:refnum<vi>)
            n385 = control-ref of="Sweep AO"() -> (w826:refnum<vi>)
            n386 = control-ref of="PS Waveform"() -> (w829:refnum<vi>)
            n387 = Bundle By Name(cluster=w828, "References.Graphs.AI Graph"=w834, "References.Graphs.AO Graph"=w833, "References.Graphs.REF Graph"=w822, "References.Graphs.Lockin 1"=w832, "References.Graphs.Lockin 2"=w831, "References.Graphs.Lockin XY"=w830, "References.Graphs.Sweep X Graph"=w823, "References.Graphs.Sweep Y Graph"=w824, "References.Graphs.Sweep AI Graph"=w825, "References.Graphs.Sweep AO Graph"=w826, "References.Graphs.PS WFGraph"=w829) -> (w827:T65)
            n388 = call <vilib>:"Add State(s) to Queue__jki_lib_state_machine.vi"("State(s) in (\"\")"=w838) -> ("States Out"=w837:string)  [unwired: 14 in]
          }
          frame "Data: Waveform Legends" {
            n389 = Unbundle By Name(w862) -> ("getAll.Waveforms.AI"=w861:waveform(dbl)[], "getAll.Waveforms.AO"=w860:waveform(dbl)[], "getAll.Waveforms.REF_X"=w843:waveform(dbl)[])
            n390 = Array Size(array=w861) -> (size(s)=w856:i32)
            n391 = Array Size(array=w860) -> (size(s)=w858:i32)
            n392 = Array Size(array=w843) -> (size(s)=w840:i32)
            n393 = call "Is Value Changed.vim"("value"=w840) -> ("changed or first call?"=w839:bool)
            n394 = call "Is Value Changed.vim"("value"=w856) -> ("changed or first call?"=w855:bool)
            n395 = call "Is Value Changed.vim"("value"=w858) -> ("changed or first call?"=w857:bool)
            n396 = Select(t="UI: Update AI Waveform Graphs Legends\nUI: Update AI Waveform Graphs Colors", s=w855, f="") -> (s? t:f=w845:string)
            n397 = Select(t="UI: Update AO Waveform Graphs Legends\nUI: Update AO Waveform Graphs Colors", s=w857, f="") -> (s? t:f=w846:string)
            n398 = Select(t="UI: Update REF Waveform Graphs Legends\nUI: Update REF Waveform Graphs Colors", s=w839, f="") -> (s? t:f=w841:string)
            n399 = call <vilib>:"Add State(s) to Queue__jki_lib_state_machine.vi"("State(s) in Front (\"\")"=w845, "State(s) in (\"\")"=w846, "State(s) at Back (\"\")"=w841) -> ("States Out"=w848:string)  [unwired: 12 in]
            n400 = call <vilib>:"Add State(s) to Queue__jki_lib_state_machine.vi"("State(s) in Front (\"\")"="UI: Defer Panel Updates >> TRUE" ("State(s) in Front (\"\")"), "State(s) in (\"\")"=w848, "State(s) at Back (\"\")"="UI: Defer Panel Updates >> FALSE" ("State(s) in Front (\"\")")) -> ("States Out"=w849:string)  [unwired: 12 in]
            n401 = Empty String/Path?(string/path=w848) -> (empty?=w852:bool)
            n402 = Select(t=w848, s=w852, f=w849) -> (s? t:f=w847:string)
            n403 = call <vilib>:"Add State(s) to Queue__jki_lib_state_machine.vi"("State(s) in Front (\"\")"=w847, "State(s) in (\"\")"=w867) -> ("States Out"=w866:string)  [unwired: 13 in]
          }
          frame "Data: Wait" {
            # "Data: wait.\n(wait for X ms)"
            n404 = Scan From String(input string=w868, default 1=u32 0 ("milliseconds to wait")) -> (output 1=w869:u32)  [unwired: 3 in, 3 out]
            n405 = Wait (ms)(milliseconds to wait=w869) -> ()  [unwired: 1 out]
            n406 = call <vilib>:"Add State(s) to Queue__jki_lib_state_machine.vi"("State(s) in (\"\")"=w875) -> ("States Out"=w874:string)  [unwired: 14 in]
          }
          frame "Data: Cleanup" {
            # "Cleanup any data and references, here.\n(this is called automatically, by the Macro: Exit)"
            n407 = Unbundle By Name(w877) -> ("Core.Current VI Reference"=w880:refnum<vi>)
            n408 = Close Reference(reference=w880, error in (no error)=w879) -> (error out=w878:errorcluster)
            n409 = call <vilib>:"Add State(s) to Queue__jki_lib_state_machine.vi"("State(s) in (\"\")"=w882) -> ("States Out"=w881:string)  [unwired: 14 in]
          }
          frame "---------- Configuration ----------" {
            # "Do not put any code in this frame.\n(It is a separator no-op. You can make a copy of this frame to create a new Data frame)"
            n410 = call <vilib>:"Add State(s) to Queue__jki_lib_state_machine.vi"("State(s) in (\"\")"=w887) -> ("States Out"=w886:string)  [unwired: 14 in]
          }
          frame "Configuration: Initialize" {
            # "Do not put any code in this frame.\n(It is a separator no-op. You can make a copy of this frame to create a new Data frame)"
            n411 = Unbundle By Name(w897) -> ("Lockin"=w896:refnum<class "Instrument.Lockin.lvclass">)
            n412 = call <vilib>:"GetName.vi"("error in (no error)"=w895, "SMO"=w896) -> ("error out"=w893:errorcluster, "Name"=w894:string)  [unwired: 6 in, 2 out]
            n413 = call <userlib>:"Default Path.vi"("error in (no error)"=w893, "Folder Name [Application Name]"=w894) -> ("error out"=w890:errorcluster, "Configuration out"=w892:refnum<class "Configuration.lvclass">)  [unwired: 8 in]
            n414 = call <userlib>:"Write Section.vi"("error in (no error)"=w890, "Section"="UI", "Configuration in"=w892) -> ("error out"=w889:errorcluster, "Configuration out"=w891:refnum<class "Configuration.lvclass">)  [unwired: 7 in]
            n415 = Bundle By Name(cluster=w897, "Configuration"=w891) -> (w898:T65)
            n416 = call <vilib>:"Add State(s) to Queue__jki_lib_state_machine.vi"("State(s) in (\"\")"=w901) -> ("States Out"=w900:string)  [unwired: 14 in]
          }
          frame "Configuration: Write File" {
            # "Do not put any code in this frame.\n(It is a separator no-op. You can make a copy of this frame to create a new Data frame)"
            n417 = Unbundle By Name(w907) -> ("Configuration"=w902:refnum<class "Configuration.lvclass">, "UI Config"=w903:T46)
            n418 = call <userlib>:"Write Configuration.vi"("error in (no error)"=w904, "Variant"=w903, "Configuration in"=w902) -> ("error out"=w906:errorcluster, "Configuration out"=w905:refnum<class "Configuration.lvclass">)  [unwired: 7 in]
            n419 = Bundle By Name(cluster=w907, "Configuration"=w905) -> (w908:T65)
            n420 = call <vilib>:"Add State(s) to Queue__jki_lib_state_machine.vi"("State(s) in (\"\")"=w911) -> ("States Out"=w910:string)  [unwired: 14 in]
          }
          frame "Configuration: Read File" {
            # "Do not put any code in this frame.\n(It is a separator no-op. You can make a copy of this frame to create a new Data frame)"
            n421 = Unbundle By Name(w920) -> ("Configuration"=w912:refnum<class "Configuration.lvclass">, "UI Config"=w914:T46)
            n422 = call <userlib>:"Read Configuration.vi"("INI Fomatted Cluster Type"=w914, "error in (no error)"=w916, "Configuration in"=w912) -> ("error out"=w918:errorcluster, "Configuration"=w919:variant, "Configuration out"=w917:refnum<class "Configuration.lvclass">)  [unwired: 6 in]
            n423 = Variant To Data(error in=w918, type=w914, Variant=w919) -> (data=w913:T46, error out=w915:errorcluster)
            n424 = Bundle By Name(cluster=w920, "Configuration"=w917, "UI Config"=w913) -> (w921:T65)
            n425 = call <vilib>:"Add State(s) to Queue__jki_lib_state_machine.vi"("State(s) in (\"\")"=w924) -> ("States Out"=w923:string)  [unwired: 14 in]
          }
          frame "---------- UI ----------" {
            # "Do not put any code in this frame.\n(It is a separator no-op. You can make a copy of this frame to create a new UI frame)"
            n426 = call <vilib>:"Add State(s) to Queue__jki_lib_state_machine.vi"("State(s) in (\"\")"=w929) -> ("States Out"=w928:string)  [unwired: 14 in]
          }
          frame "UI: Initialize" {
            # "size window to decoration box on front panel"
            # "Initialize the User Interface here.\n(this is called automatically, by the Macro: Init)"
            n427 = call "Application Version.vi"() -> ("Version"=→"Version" →"Application Version":string)
            n428 = call <userlib>:"Fit VI window to Largest Dec__ogtk.vi"("error in (no error)"=w938, "border spacing (2 px)"=-4) -> ("error out"=w937:errorcluster)  [unwired: 4 in, 1 out]
            n429 = local write "Sampling Status"(u32 6618880) -> ()
            n430 = call <vilib>:"Build State String with Arguments__JKI_lib_State_Machine.vi"("Arguments (\"\")"="Initializing..." ("Status"), "State"="UI: Update Status") -> ("State with Arguments"=w932:string)  [unwired: 4 in]
            n431 = call <vilib>:"Add State(s) to Queue__jki_lib_state_machine.vi"("State(s) in Front (\"\")"=w932, "State(s) in (\"\")"=w941) -> ("States Out"=w940:string)  [unwired: 13 in]
          }
          frame "UI: Cursor Set" {
            # "Argument"
            # "Initialize the User Interface, here.\n(this is called automatically, by the Macro: Init)"
            n432 = disable-structure shown="Default" {
              disable-tunnel: w944 -> [w949 w952]
              disable-tunnel: [w949 w951] -> w943
              disable-tunnel: w942 -> [_ w950]
              frame condition #0 {
              }
              frame condition #1 (active) {
                n433 = case shown="\"Idle\", Default" w950 {
                  tunnel: w952 -> [w954 w956]
                  tunnel: [w953 w955] -> w951
                  frame "Idle", Default {
                    n434 = call <vilib>:"Unset Busy.vi"("error in (no error)"=w954) -> ("error out"=w953:errorcluster)  [unwired: 10 in]
                  }
                  frame "Busy" {
                    n435 = call <vilib>:"Set Busy.vi"("error in (no error)"=w956) -> ("error out"=w955:errorcluster)  [unwired: 9 in, 1 out]
                  }
                }
              }
            }
            n436 = call <vilib>:"Add State(s) to Queue__jki_lib_state_machine.vi"("State(s) in (\"\")"=w948) -> ("States Out"=w947:string)  [unwired: 14 in]
          }
          frame "UI: Front Panel State" {
            # "Argument"
            # "Set Front Panel Open or Closed\n(Usage: \"UI: Front Panel State >> Open|Close\")"
            n437 = Unbundle By Name(w960) -> ("Core.Current VI Reference"=w959:refnum<vi>)
            n438 = disable-structure shown="Default" {
              disable-tunnel: w962 -> [w968 w991]
              disable-tunnel: [w967 w991] -> w961
              disable-tunnel: w959 -> [w966 _]
              disable-tunnel: w958 -> [w965 _]
              frame condition #0 (active) {
                n439 = case shown="\"Close\"" w965 {
                  tunnel: w968 -> [w972 w985]
                  tunnel: [w974 w986] -> w967
                  tunnel: w966 -> [w973 w983]
                  frame "Open", Default {
                    n440 = property class="VI"(reference=w973, error in=w972) -> (reference out=w970:refnum<vi>, error out=w971:errorcluster, "FP.State"=w969:T35)
                    n441 = case shown="\"Closed\"" w969 {
                      tunnel: [w977 w980] -> w974
                      tunnel: w971 -> [w976 w980]
                      tunnel: w970 -> [w975 _]
                      frame "Closed" {
                        n442 = invoke class="VI" method="FP.Open"(reference=w975, error in=w976, "Activate"=TRUE, "State"=T35."Standard") -> (error out=w977:errorcluster)  [unwired: 1 in, 4 out]
                      }
                      frame Default {
                      }
                    }
                  }
                  frame "Close" {
                    n443 = property class="VI"(reference=w983, error in=w985) -> (reference out=w982:refnum<vi>, error out=w984:errorcluster, "FP.State"=w981:T35)
                    n444 = case shown="Default" w981 {
                      tunnel: [w987 w990] -> w986
                      tunnel: w984 -> [w987 w989]
                      tunnel: w982 -> [_ w988]
                      frame "Invalid", "Closed" {
                      }
                      frame Default {
                        n445 = invoke class="VI" method="FP.Close"(reference=w988, error in=w989) -> (error out=w990:errorcluster)  [unwired: 1 in, 2 out]
                      }
                    }
                  }
                }
              }
              frame condition #1 {
              }
            }
            n446 = call <vilib>:"Add State(s) to Queue__jki_lib_state_machine.vi"("State(s) in (\"\")"=w964) -> ("States Out"=w963:string)  [unwired: 14 in]
          }
          frame "UI: Defer Panel Updates" {
            # "Do not put any code in this frame.\n(It is a separator no-op. You can make a copy of this frame to create a new UI frame)"
            n447 = Unbundle By Name(w996) -> ("Front Panel"=w994:refnum<vi>)
            n448 = Scan From String(input string=w995, default 1=FALSE) -> (output 1=w993:bool)  [unwired: 3 in, 3 out]
            n449 = property class="Pnl"(reference=w994, "Defer Panel Updates"=w993) -> ()  [unwired: 1 in, 2 out]
            n450 = call <vilib>:"Add State(s) to Queue__jki_lib_state_machine.vi"("State(s) in (\"\")"=w1000) -> ("States Out"=w999:string)  [unwired: 14 in]
          }
          frame "UI: Set Left Tab" {
            # "Do not put any code in this frame.\n(It is a separator no-op. You can make a copy of this frame to create a new UI frame)"
            n451 = Scan From String(input string=w1003, default 1=T1."AO/AI/REF" ("Left Tab")) -> (output 1=w1002:T1)  [unwired: 3 in, 3 out]
            n452 = local write "Left Tab"(w1002) -> ()
            n453 = call <vilib>:"Add State(s) to Queue__jki_lib_state_machine.vi"("State(s) in (\"\")"=w1008) -> ("States Out"=w1007:string)  [unwired: 14 in]
          }
          frame "UI: Set Right Tab" {
            # "Do not put any code in this frame.\n(It is a separator no-op. You can make a copy of this frame to create a new UI frame)"
            n454 = Scan From String(input string=w1011, default 1=T25."AO/AI Graphs" ("Right Tab")) -> (output 1=w1010:T25)  [unwired: 3 in, 3 out]
            n455 = local write "Right Tab"(w1010) -> ()
            n456 = call <vilib>:"Add State(s) to Queue__jki_lib_state_machine.vi"("State(s) in (\"\")"=w1016) -> ("States Out"=w1015:string)  [unwired: 14 in]
          }
          frame "UI: Init Scroll Bars" {
            w1018 = u32[] [0] ("Index Values")
            w1017 = u32 0 ("Legend:Scroll Position")
            # "UI: Init Scroll Bars.\n(Scroll to the top)"
            n457 = property on="Lockin 1" class="WFGraph (strict)"("LegScrollPos"=w1017) -> ()  [unwired: 2 in, 2 out]
            n458 = property on="Lockin 2" class="WFGraph (strict)"("LegScrollPos"=w1017) -> ()  [unwired: 2 in, 2 out]
            n459 = property on="AI Graph" class="WFGraph (strict)"("LegScrollPos"=w1017) -> ()  [unwired: 2 in, 2 out]
            n460 = property on="AO Graph" class="WFGraph (strict)"("LegScrollPos"=w1017) -> ()  [unwired: 2 in, 2 out]
            n461 = property on="REF Graph" class="WFGraph (strict)"("LegScrollPos"=w1017) -> ()  [unwired: 2 in, 2 out]
            n462 = property on="Lockin XY" class="XYGraph (strict)"("LegScrollPos"=w1017) -> ()  [unwired: 2 in, 2 out]
            n463 = property on="AO Channels" class="Arr (strict)"("Index Values"=w1018) -> ()  [unwired: 2 in, 2 out]
            n464 = property on="DAQ Config" class="Arr (strict)"("Index Values"=w1018) -> ()  [unwired: 2 in, 2 out]
            n465 = property on="Sweep AI" class="WFGraph (strict)"("LegScrollPos"=w1017) -> ()  [unwired: 2 in, 2 out]
            n466 = property on="Sweep AO" class="WFGraph (strict)"("LegScrollPos"=w1017) -> ()  [unwired: 2 in, 2 out]
            n467 = property on="Sweep X" class="WFGraph (strict)"("LegScrollPos"=w1017) -> ()  [unwired: 2 in, 2 out]
            n468 = property on="Sweep Y" class="WFGraph (strict)"("LegScrollPos"=w1017) -> ()  [unwired: 2 in, 2 out]
            n469 = property on="PS Waveform" class="WFGraph (strict)"("LegScrollPos"=w1017) -> ()  [unwired: 2 in, 2 out]
            n470 = property on="AI Channels" class="Arr (strict)"("Index Values"=w1018) -> ()  [unwired: 2 in, 2 out]
            n471 = call <vilib>:"Add State(s) to Queue__jki_lib_state_machine.vi"("State(s) in (\"\")"=w1023) -> ("States Out"=w1022:string)  [unwired: 14 in]
          }
          frame "UI: Update Status" {
            # "UI: Update Status.\n()"
            n472 = case shown="Default" w1024 {
              selector: w1024 -> [w1030 _]
              frame Default {
                "String" <- w1030
              }
              frame "" {
              }
            }
            n473 = call <vilib>:"Add State(s) to Queue__jki_lib_state_machine.vi"("State(s) in (\"\")"=w1029) -> ("States Out"=w1028:string)  [unwired: 14 in]
          }
          frame "UI: Cluster to UI" {
            # "Initialize the UI elements from data wire\n(this is called automatically, by the Macro: Init)"
            n474 = Unbundle By Name(w1039) -> ("UI Config.Channels.Cfg_AO"=w1054:T6, "UI Config.Channels.Cfg_AI"=w1052:T4, "UI Config.Channels.Cfg_REF"=w1053:T2, "UI Config.DAQ.Configuration"=w1046:T9, "UI Config.DAQ.cfg.Sampling.Sampling.Fs"=w1035:dbl, "UI Config.DAQ.cfg.Sampling.Sampling.#s"=w1034:i32, "UI Config.DAQ.cfg.Sampling.Fs Mode"=w1031:T15, "UI Config.DAQ.cfg.Sampling.Fs Multiplier"=w1047:dbl, "UI Config.DAQ.cfg.Sampling.Refresh Rate (Hz)"=w1048:dbl, "UI Config.DAQ.cfg.Sampling.Fs.Output"=w1038:dbl, "UI Config.DAQ.cfg.Sampling.Decimation.PreDSP"=w1044:i32, "UI Config.DAQ.Simulation mode"=w1045:T16, "UI Config.PreFilter.60 Hz"=w1051:bool, "UI Config.PreFilter.Low Pass"=w1050:bool, "UI Config.PreFilter.Low Pass Cutoff (Hz)"=w1049:dbl, "UI Config.Amplifers.Offset_AI"=w1032:T17, "UI Config.Amplifers.Gain_AI"=w1037:T17, "UI Config.Amplifers.Gain_AO"=w1033:T17, "UI Config.Sweep.sweepTime"=w1040:dbl, "UI Config.Sweep.initialWaitTime"=w1041:dbl, "UI Config.Sweep.returnToStart"=w1042:bool, "UI Config.Sweep.sweepChannels"=w1043:T20)
            n475 = local write "Fs (S/s)"(w1035) -> ()
            n476 = local write "#s (S)"(w1034) -> ()
            n477 = local write "Input Offsets"(w1032) -> ()
            n478 = local write "Input Gain"(w1037) -> ()
            n479 = local write "Output Gain"(w1033) -> ()
            n480 = local write "Fs Output (S/s)"(w1038) -> ()
            n481 = local write "Fs (S/s) (buffer)"(w1035) -> ()
            n482 = local write "#s (S) (buffer)"(w1034) -> ()
            n483 = local write "AO Channels"(w1054) -> ()
            n484 = local write "AI Channels"(w1052) -> ()
            n485 = local write "REF Channels"(w1053) -> ()
            n486 = local write "DAQ Config"(w1046) -> ()
            n487 = local write "Fs Multiplier"(w1047) -> ()
            n488 = local write "Refresh Rate (Hz)"(w1048) -> ()
            n489 = local write "Decimation (pre DSP)"(w1044) -> ()
            n490 = local write "AI Simulation mode"(w1045) -> ()
            n491 = local write "Line"(w1051) -> ()
            n492 = local write "Lowpass"(w1050) -> ()
            n493 = local write "LP f (Hz)"(w1049) -> ()
            n494 = local write "Sweep Time (s)"(w1040) -> ()
            n495 = local write "Initial Wait (s)"(w1041) -> ()
            n496 = local write "Return to Start?"(w1042) -> ()
            n497 = local write "Sweep Channels"(w1043) -> ()
            n498 = local write "Fs Mode"(w1031) -> ()
            n499 = call <vilib>:"Add State(s) to Queue__jki_lib_state_machine.vi"("State(s) in Front (\"\")"="" ("State(s) in Front (\"\")"), "State(s) in (\"\")"=w1058) -> ("States Out"=w1057:string)  [unwired: 13 in]
          }
          frame "UI: Cluster to UI 2" {
            # "Initialize the UI elements from data wire (2)\n(this is called automatically by Macro: Init)"
            n500 = Unbundle By Name(w1067) -> ("UI Config.Limit Amplitude.Limit?"=w1066:bool, "UI Config.Limit Amplitude.Limit (V)"=w1065:dbl, "UI Config.Limit DC.Limit?"=w1062:bool, "UI Config.Limit DC.Limit (V)"=w1061:dbl, "UI Config.Link Frequencies.Link?"=w1063:bool, "UI Config.Link Frequencies.Frequency (Hz)"=w1064:dbl, "UI Config.Plot.Display 1"=w1060:T26, "UI Config.Plot.Display 2"=w1059:T26)
            n501 = local write "Limit DC?"(w1062) -> ()
            n502 = local write "Display 1"(w1060) -> ()
            n503 = local write "Display 2"(w1059) -> ()
            n504 = local write "Limit AC?"(w1066) -> ()
            n505 = local write "Link f?"(w1063) -> ()
            n506 = local write "AO DC Limit"(w1061) -> ()
            n507 = local write "f link (Hz)"(w1064) -> ()
            n508 = local write "AC Limit"(w1065) -> ()
            n509 = call <vilib>:"Add State(s) to Queue__jki_lib_state_machine.vi"("State(s) in (\"\")"=w1071) -> ("States Out"=w1070:string)  [unwired: 14 in]
          }
          frame "UI: UI to Cluster" {
            # "Write UI elements to data wire\n(this is called automatically, by the Macro: Save Configuration)"
            n510 = local read "AO Channels"() -> (w1094:T6)
            n511 = local read "AI Channels"() -> (w1092:T4)
            n512 = local read "REF Channels"() -> (w1093:T2)
            n513 = local read "DAQ Config"() -> (w1085:T9)
            n514 = local read "Fs Mode"() -> (w1088:T15)
            n515 = local read "Fs Multiplier"() -> (w1086:dbl)
            n516 = local read "Refresh Rate (Hz)"() -> (w1087:dbl)
            n517 = local read "Decimation (pre DSP)"() -> (w1083:i32)
            n518 = local read "AI Simulation mode"() -> (w1084:T16)
            n519 = local read "Line"() -> (w1091:bool)
            n520 = local read "Lowpass"() -> (w1090:bool)
            n521 = local read "LP f (Hz)"() -> (w1089:dbl)
            n522 = local read "Sweep Time (s)"() -> (w1079:dbl)
            n523 = local read "Initial Wait (s)"() -> (w1080:dbl)
            n524 = local read "Return to Start?"() -> (w1081:bool)
            n525 = local read "Sweep Channels"() -> (w1082:T20)
            n526 = local read "Fs (S/s)"() -> (w1074:dbl)
            n527 = local read "#s (S)"() -> (w1075:i32)
            n528 = local read "Fs Output (S/s)"() -> (w1073:dbl)
            n529 = local read "Input Offsets"() -> (w1076:T17)
            n530 = local read "Input Gain"() -> (w1078:T17)
            n531 = local read "Output Gain"() -> (w1077:T17)
            n532 = Bundle By Name(cluster=w1095, "UI Config.Channels.Cfg_AO"=w1094, "UI Config.Channels.Cfg_AI"=w1092, "UI Config.Channels.Cfg_REF"=w1093, "UI Config.DAQ.Configuration"=w1085, "UI Config.DAQ.cfg.Sampling.Sampling.Fs"=w1074, "UI Config.DAQ.cfg.Sampling.Sampling.#s"=w1075, "UI Config.DAQ.cfg.Sampling.Fs Mode"=w1088, "UI Config.DAQ.cfg.Sampling.Fs Multiplier"=w1086, "UI Config.DAQ.cfg.Sampling.Refresh Rate (Hz)"=w1087, "UI Config.DAQ.cfg.Sampling.Fs.Output"=w1073, "UI Config.DAQ.cfg.Sampling.Decimation.PreDSP"=w1083, "UI Config.DAQ.Simulation mode"=w1084, "UI Config.PreFilter.60 Hz"=w1091, "UI Config.PreFilter.Low Pass"=w1090, "UI Config.PreFilter.Low Pass Cutoff (Hz)"=w1089, "UI Config.Amplifers.Offset_AI"=w1076, "UI Config.Amplifers.Gain_AI"=w1078, "UI Config.Amplifers.Gain_AO"=w1077, "UI Config.Sweep.sweepTime"=w1079, "UI Config.Sweep.initialWaitTime"=w1080, "UI Config.Sweep.returnToStart"=w1081, "UI Config.Sweep.sweepChannels"=w1082) -> (w1096:T65)
            n533 = call <vilib>:"Add State(s) to Queue__jki_lib_state_machine.vi"("State(s) in Front (\"\")"="" ("State(s) in Front (\"\")"), "State(s) in (\"\")"=w1100) -> ("States Out"=w1099:string)  [unwired: 13 in]
          }
          frame "UI: UI to Cluster 2" {
            # "Write UI elements to data wire (2)\n(this is called automatically, by the Macro: Save Configuration)"
            n534 = local read "Limit DC?"() -> (w1108:bool)
            n535 = local read "Limit AC?"() -> (w1110:bool)
            n536 = local read "Link f?"() -> (w1106:bool)
            n537 = local read "Display 1"() -> (w1102:T26)
            n538 = local read "Display 2"() -> (w1101:T26)
            n539 = local read "AO DC Limit"() -> (w1107:dbl)
            n540 = local read "f link (Hz)"() -> (w1105:dbl)
            n541 = local read "AC Limit"() -> (w1109:dbl)
            n542 = Bundle By Name(cluster=w1103, "UI Config.Limit Amplitude.Limit?"=w1110, "UI Config.Limit Amplitude.Limit (V)"=w1109, "UI Config.Limit DC.Limit?"=w1108, "UI Config.Limit DC.Limit (V)"=w1107, "UI Config.Link Frequencies.Link?"=w1106, "UI Config.Link Frequencies.Frequency (Hz)"=w1105, "UI Config.Plot.Display 1"=w1102, "UI Config.Plot.Display 2"=w1101) -> (w1104:T65)
            n543 = call <vilib>:"Add State(s) to Queue__jki_lib_state_machine.vi"("State(s) in (\"\")"=w1114) -> ("States Out"=w1113:string)  [unwired: 14 in]
          }
          frame "UI: Reinit To Default" {
            # "UI: Reinit To Default.\n(I)"
            n544 = Unbundle By Name(w1115) -> ("References.Booleans"=w1117:T62, "References.Graphs.Lockin 1"=w1119:refnum<vi>, "References.Graphs.Lockin 2"=w1118:refnum<vi>)
            n545 = Cluster To Array(cluster=w1117) -> (array=w1116:refnum<vi>[])
            n546 = for {
              tunnel: w1116 -> [w1124] mode=indexing
              n547 = invoke on="Invoke Node" class="Bool (strict)" method="Reinit To Default"(reference=w1124) -> ()  [unwired: 2 in, 3 out]
            }
            n548 = invoke on="Invoke Node" class="WFGraph (strict)" method="Reinit To Default"(reference=w1119) -> ()  [unwired: 2 in, 3 out]
            n549 = invoke on="Invoke Node" class="WFGraph (strict)" method="Reinit To Default"(reference=w1118) -> ()  [unwired: 2 in, 3 out]
            n550 = call <vilib>:"Add State(s) to Queue__jki_lib_state_machine.vi"("State(s) in (\"\")"=w1123) -> ("States Out"=w1122:string)  [unwired: 14 in]
          }
          frame "UI: Disable Buttons" {
            # "UI: Disable Buttons\n(Disable all booleans)"
            n551 = Unbundle By Name(w1126) -> ("References.Booleans"=w1127:T62)
            n552 = Cluster To Array(cluster=w1127) -> (array=w1125:refnum<vi>[])
            n553 = for {
              tunnel: w1125 -> [w1132] mode=indexing
              n554 = property class="Bool (strict)"(reference=w1132, "DisabledEnum"=T36."Disabled and Grayed Out" ("Disabled")) -> ()  [unwired: 1 in, 2 out]
            }
            n555 = call <vilib>:"Add State(s) to Queue__jki_lib_state_machine.vi"("State(s) in (\"\")"=w1131) -> ("States Out"=w1130:string)  [unwired: 14 in]
          }
          frame "UI: Enable Buttons" {
            # "UI: Enable Buttons.\n(Enable booleans after SMO starts.)"
            n556 = Unbundle By Name(w1136) -> ("References.Booleans"=w1135:T62)
            n557 = Cluster To Array(cluster=w1135) -> (array=w1134:refnum<vi>[])
            n558 = for {
              tunnel: w1134 -> [w1141] mode=indexing
              n559 = property class="Bool (strict)"(reference=w1141, "DisabledEnum"=T36."Enabled" ("Disabled")) -> ()  [unwired: 1 in, 2 out]
            }
            n560 = call <vilib>:"Add State(s) to Queue__jki_lib_state_machine.vi"("State(s) in (\"\")"=w1140) -> ("States Out"=w1139:string)  [unwired: 14 in]
          }
          frame "UI: Update Booleans" {
            # "UI: Update Booleans.\n(Call in response to state upate)"
            n561 = Unbundle By Name(w1145) -> ("DAQ state"=w1144:T33, "References.Booleans.Start"=w1151:refnum<vi>, "References.Booleans.Pause"=w1150:refnum<vi>, "References.Booleans.Reset"=w1152:refnum<vi>, "References.Booleans.Trigger"=w1149:refnum<vi>, "References.Booleans.Start Sweep"=w1148:refnum<vi>, "References.Booleans.Stop Sweep"=w1146:refnum<vi>)
            n562 = case shown="\"idle\", Default" w1144 {
              tunnel: w1152 -> [w1163 w1169 w1172 w1175 _]
              tunnel: w1151 -> [w1164 w1166 w1173 w1176 _]
              tunnel: w1150 -> [_ _ _ _ _]
              tunnel: w1149 -> [w1162 _ w1171 _ _]
              tunnel: w1148 -> [_ w1168 _ _ _]
              tunnel: [w1161 w1170 w1174 w1178 _] -> w1147
              tunnel: [_ w1165 _ w1177 _] -> w1143
              tunnel: w1146 -> [_ w1167 _ _ _]
              frame "idle", Default {
                n563 = Build Array(w1164, w1163, w1162) -> (w1161:refnum<vi>[])
              }
              frame "started" {
                n564 = Build Array(w1166) -> (w1165:refnum<vi>[])
                n565 = Build Array(w1169, w1168, w1167) -> (w1170:refnum<vi>[])
              }
              frame "stopped" {
                n566 = Build Array(w1173, w1172, w1171) -> (w1174:refnum<vi>[])
              }
              frame "created" {
                n567 = Build Array(w1176) -> (w1177:refnum<vi>[])
                n568 = Build Array(w1175) -> (w1178:refnum<vi>[])
              }
              frame "sweeping" {
              }
            }
            n569 = for {
              tunnel: w1143 -> [w1157] mode=indexing
              n570 = property class="Bool (strict)"(reference=w1157, "Value"=TRUE) -> ()  [unwired: 1 in, 2 out]
            }
            n571 = for {
              tunnel: w1147 -> [w1159] mode=indexing
              n572 = property class="Bool (strict)"(reference=w1159, "Value"=FALSE) -> ()  [unwired: 1 in, 2 out]
            }
            n573 = call <vilib>:"Add State(s) to Queue__jki_lib_state_machine.vi"("State(s) in (\"\")"=w1156) -> ("States Out"=w1155:string)  [unwired: 14 in]
          }
          frame "UI: AI Graphs Plot Visibility" {
            n574 = Unbundle By Name(w1183) -> ("References.Graphs.AI Graph"=w1182:refnum<vi>, "References.Graphs.Sweep AI Graph"=w1179:refnum<vi>)
            n575 = case shown="\"None\", Default" w1181 {
              tunnel: [FALSE TRUE] -> w1180
              frame "None", Default {
              }
              frame "ALL" {
              }
            }
            n576 = call-poly "Set All Plot Visibility.vi"("error in (no error)"=w1184, "All Visible?"=w1180, "WFGraph in"=w1179) -> ("error out"=w1186:errorcluster)  [unwired: 8 in]
            n577 = call-poly "Set All Plot Visibility.vi"("error in (no error)"=w1186, "All Visible?"=w1180, "WFGraph in"=w1182) -> ("error out"=w1185:errorcluster)  [unwired: 8 in]
            n578 = call <vilib>:"Add State(s) to Queue__jki_lib_state_machine.vi"("State(s) in (\"\")"=w1189) -> ("States Out"=w1188:string)  [unwired: 14 in]
          }
          frame "UI: AO Graphs Plot Visibility" {
            n579 = Unbundle By Name(w1197) -> ("References.Graphs.AO Graph"=w1196:refnum<vi>, "References.Graphs.Sweep AO Graph"=w1193:refnum<vi>)
            n580 = case shown="\"ALL\"" w1195 {
              tunnel: [FALSE TRUE] -> w1192
              frame "None", Default {
              }
              frame "ALL" {
              }
            }
            n581 = call-poly "Set All Plot Visibility.vi"("error in (no error)"=w1198, "All Visible?"=w1192, "WFGraph in"=w1193) -> ("error out"=w1199:errorcluster)  [unwired: 8 in]
            n582 = call-poly "Set All Plot Visibility.vi"("error in (no error)"=w1199, "All Visible?"=w1192, "WFGraph in"=w1196) -> ("error out"=w1194:errorcluster)  [unwired: 8 in]
            n583 = call <vilib>:"Add State(s) to Queue__jki_lib_state_machine.vi"("State(s) in (\"\")"=w1202) -> ("States Out"=w1201:string)  [unwired: 14 in]
          }
          frame "UI: REF Graphs Plot Visibility" {
            n584 = Unbundle By Name(w1209) -> ("References.Graphs.REF Graph"=w1206:refnum<vi>)
            n585 = case shown="\"ALL\"" w1208 {
              tunnel: [FALSE TRUE] -> w1205
              frame "None", Default {
              }
              frame "ALL" {
              }
            }
            n586 = call-poly "Set All Plot Visibility.vi"("error in (no error)"=w1210, "All Visible?"=w1205, "WFGraph in"=w1206) -> ("error out"=w1207:errorcluster)  [unwired: 8 in]
            n587 = call <vilib>:"Add State(s) to Queue__jki_lib_state_machine.vi"("State(s) in (\"\")"=w1213) -> ("States Out"=w1212:string)  [unwired: 14 in]
          }
          frame "UI: Lockin Graphs Plot Visibility" {
            n588 = Unbundle By Name(w1227) -> ("References.Graphs.Lockin 1"=w1218:refnum<vi>, "References.Graphs.Lockin 2"=w1219:refnum<vi>, "References.Graphs.Lockin XY"=w1220:refnum<vi>, "References.Graphs.Sweep X Graph"=w1217:refnum<vi>, "References.Graphs.Sweep Y Graph"=w1216:refnum<vi>)
            n589 = case shown="\"ALL\"" w1226 {
              tunnel: [FALSE TRUE] -> w1221
              frame "None", Default {
              }
              frame "ALL" {
              }
            }
            n590 = call-poly "Set All Plot Visibility.vi"("error in (no error)"=w1228, "All Visible?"=w1221, "WFGraph in"=w1216) -> ("error out"=w1229:errorcluster)  [unwired: 8 in]
            n591 = call-poly "Set All Plot Visibility.vi"("error in (no error)"=w1229, "All Visible?"=w1221, "WFGraph in"=w1217) -> ("error out"=w1225:errorcluster)  [unwired: 8 in]
            n592 = call-poly "Set All Plot Visibility.vi"("error in (no error)"=w1225, "All Visible?"=w1221, "XYGraph in"=w1220) -> ("error out"=w1224:errorcluster)  [unwired: 7 in, 1 out]
            n593 = call-poly "Set All Plot Visibility.vi"("error in (no error)"=w1224, "All Visible?"=w1221, "WFGraph in"=w1219) -> ("error out"=w1223:errorcluster)  [unwired: 8 in]
            n594 = call-poly "Set All Plot Visibility.vi"("error in (no error)"=w1223, "All Visible?"=w1221, "WFGraph in"=w1218) -> ("error out"=w1222:errorcluster)  [unwired: 8 in]
            n595 = call <vilib>:"Add State(s) to Queue__jki_lib_state_machine.vi"("State(s) in (\"\")"=w1232) -> ("States Out"=w1231:string)  [unwired: 14 in]
          }
          frame "UI: Get Plot Visibility" {
            n596 = Unbundle By Name(w1247) -> ("References.Graphs.AI Graph"=w1244:refnum<vi>, "References.Graphs.AO Graph"=w1243:refnum<vi>, "References.Graphs.Lockin 1"=w1245:refnum<vi>)
            n597 = call-poly "Get Plot Visibility.vi"("error in (no error)"=w1238, "WFGraph in"=w1244) -> ("error out"=w1239:errorcluster, "Plot.Visible"=w1237:bool[])  [unwired: 8 in]
            n598 = call-poly "Get Plot Visibility.vi"("error in (no error)"=w1238, "WFGraph in"=w1245) -> ("error out"=w1242:errorcluster, "Plot.Visible"=w1235:bool[])  [unwired: 8 in]
            n599 = call-poly "Get Plot Visibility.vi"("error in (no error)"=w1238, "WFGraph in"=w1243) -> ("error out"=w1240:errorcluster, "Plot.Visible"=w1236:bool[])  [unwired: 8 in]
            n600 = Bundle By Name(cluster=w1247, "UI Config.Plot.visibility.AI"=w1237, "UI Config.Plot.visibility.AO"=w1236, "UI Config.Plot.visibility.Lockin"=w1235) -> (w1246:T65)
            n601 = Merge Errors(w1238, w1239, w1240, w1242) -> (w1241:errorcluster)
            n602 = call <vilib>:"Add State(s) to Queue__jki_lib_state_machine.vi"("State(s) in (\"\")"=w1250) -> ("States Out"=w1249:string)  [unwired: 14 in]
          }
          frame "UI: Set Plot Visibility" {
            n603 = Unbundle By Name(w1254) -> ("References.Graphs.AI Graph"=w1261:refnum<vi>, "UI Config.Plot.visibility.AI"=w1252:bool[], "References.Graphs.AO Graph"=w1260:refnum<vi>, "UI Config.Plot.visibility.AO"=w1253:bool[], "References.Graphs.Lockin 1"=w1262:refnum<vi>, "UI Config.Plot.visibility.Lockin"=w1251:bool[])
            n604 = call-poly "Set Plot Visibility.vi"("error in (no error)"=w1255, "Plot.Visible?"=w1252, "WFGraph in"=w1261) -> ("error out"=w1256:errorcluster)  [unwired: 8 in]
            n605 = call-poly "Set Plot Visibility.vi"("error in (no error)"=w1255, "Plot.Visible?"=w1253, "WFGraph in"=w1260) -> ("error out"=w1257:errorcluster)  [unwired: 8 in]
            n606 = call-poly "Set Plot Visibility.vi"("error in (no error)"=w1255, "Plot.Visible?"=w1251, "WFGraph in"=w1262) -> ("error out"=w1259:errorcluster)  [unwired: 8 in]
            n607 = Merge Errors(w1256, w1257, w1259) -> (w1258:errorcluster)
            n608 = call <vilib>:"Add State(s) to Queue__jki_lib_state_machine.vi"("State(s) in (\"\")"=w1265) -> ("States Out"=w1264:string)  [unwired: 14 in]
          }
          frame "UI: Sync AI Plot Visibility" {
            n609 = Unbundle By Name(w1275) -> ("References.Graphs.PS WFGraph"=w1271:refnum<vi>, "References.Graphs.Sweep AI Graph"=w1272:refnum<vi>, "References.Graphs.AI Graph"=w1273:refnum<vi>)
            n610 = call-poly "Get Plot Visibility.vi"("error in (no error)"=w1267, "WFGraph in"=w1273) -> ("error out"=w1270:errorcluster, "Plot.Visible"=w1268:bool[])  [unwired: 8 in]
            n611 = call-poly "Set Plot Visibility.vi"("error in (no error)"=w1270, "Plot.Visible?"=w1268, "WFGraph in"=w1272) -> ("error out"=w1266:errorcluster)  [unwired: 8 in]
            n612 = call-poly "Set Plot Visibility.vi"("error in (no error)"=w1267, "Plot.Visible?"=w1268, "WFGraph (WDT) in"=w1271) -> ("error out"=w1269:errorcluster)  [unwired: 8 in]
            n613 = Merge Errors(w1266, w1269) -> (w1274:errorcluster)
            n614 = call <vilib>:"Add State(s) to Queue__jki_lib_state_machine.vi"("State(s) in (\"\")"=w1278) -> ("States Out"=w1277:string)  [unwired: 14 in]
          }
          frame "UI: Sync AO Plot Visibility" {
            n615 = Unbundle By Name(w1286) -> ("References.Graphs.Sweep AO Graph"=w1285:refnum<vi>, "References.Graphs.AO Graph"=w1283:refnum<vi>)
            n616 = call-poly "Get Plot Visibility.vi"("error in (no error)"=w1281, "WFGraph in"=w1283) -> ("error out"=w1279:errorcluster, "Plot.Visible"=w1280:bool[])  [unwired: 8 in]
            n617 = call-poly "Set Plot Visibility.vi"("error in (no error)"=w1279, "Plot.Visible?"=w1280, "WFGraph in"=w1285) -> ("error out"=w1282:errorcluster)  [unwired: 8 in]
            n618 = Merge Errors(w1282) -> (w1284:errorcluster)
            n619 = call <vilib>:"Add State(s) to Queue__jki_lib_state_machine.vi"("State(s) in (\"\")"=w1289) -> ("States Out"=w1288:string)  [unwired: 14 in]
          }
          frame "UI: Sync Lockin Plot Visibility" {
            # "Do not put any code in this frame.\n(It is a separator no-op. You can make a copy of this frame to create a new UI frame)"
            n620 = Unbundle By Name(w1303) -> ("References.Graphs.Sweep X Graph"=w1297:refnum<vi>, "References.Graphs.Sweep Y Graph"=w1298:refnum<vi>, "References.Graphs.Lockin XY"=w1299:refnum<vi>, "References.Graphs.Lockin 2"=w1302:refnum<vi>, "References.Graphs.Lockin 1"=w1300:refnum<vi>)
            n621 = call-poly "Get Plot Visibility.vi"("error in (no error)"=w1291, "WFGraph in"=w1300) -> ("error out"=w1292:errorcluster, "Plot.Visible"=w1290:bool[])  [unwired: 8 in]
            n622 = call-poly "Set Plot Visibility.vi"("error in (no error)"=w1292, "Plot.Visible?"=w1290, "WFGraph in"=w1302) -> ("error out"=w1293:errorcluster)  [unwired: 8 in]
            n623 = call-poly "Set Plot Visibility.vi"("error in (no error)"=w1292, "Plot.Visible?"=w1290, "XYGraph in"=w1299) -> ("error out"=w1294:errorcluster)  [unwired: 8 in]
            n624 = call-poly "Set Plot Visibility.vi"("error in (no error)"=w1292, "Plot.Visible?"=w1290, "WFGraph in"=w1298) -> ("error out"=w1295:errorcluster)  [unwired: 8 in]
            n625 = call-poly "Set Plot Visibility.vi"("error in (no error)"=w1292, "Plot.Visible?"=w1290, "WFGraph in"=w1297) -> ("error out"=w1296:errorcluster)  [unwired: 8 in]
            n626 = Merge Errors(w1296, w1295, w1294, w1293) -> (w1301:errorcluster)
            n627 = call <vilib>:"Add State(s) to Queue__jki_lib_state_machine.vi"("State(s) in (\"\")"=w1306) -> ("States Out"=w1305:string)  [unwired: 14 in]
          }
          frame "UI: Update Waveform Graphs" {
            n628 = Unbundle By Name(w1337) -> ("UI Config.DAQ.cfg.Sampling.Sampling"=w1324:T49, "UI Config.Amplifers.Gain_AI"=w1330:T17, "getAll.Waveforms.AI"=w1318:waveform(dbl)[], "getAll.Waveforms.AO"=w1319:waveform(dbl)[], "getAll.Waveforms.REF_X"=w1320:waveform(dbl)[], "getAll.Waveforms.REF_Y"=w1328:waveform(dbl)[])
            n629 = Decrement(x="Sync Ch") -> (x-1=w1325:i32)
            n630 = for {
              tunnel: w1330 -> [w1371] mode=indexing
              tunnel: [w1370] -> w1329 mode=indexing
              n631 = Unbundle By Name(w1371) -> ("Gain"=w1370:dbl)
            }
            n632 = Interleave 1D Arrays(w1320, w1328) -> (w1317:waveform(dbl)[])
            n633 = case shown="True" "Sync?" {
              tunnel: [w1347 w1368] -> w1314
              tunnel: w1318 -> [w1347 w1367]
              tunnel: w1319 -> [w1345 w1366]
              tunnel: [w1346 w1365] -> w1315
              tunnel: [w1344 w1364] -> w1312
              tunnel: [w1345 w1363] -> w1311
              tunnel: w1316 -> [w1344 w1362]
              tunnel: w1317 -> [w1343 w1361]
              tunnel: w1316 -> [w1342 w1360]
              tunnel: [w1342 w1359] -> w1310
              tunnel: [w1343 w1358] -> w1309
              tunnel: w1325 -> [_ w1357]
              tunnel: w1316 -> [w1346 w1356]
              tunnel: w1324 -> [_ w1355]
              tunnel: [_ w1353] -> w1322
              tunnel: [_ w1351] -> w1321
              tunnel: w1320 -> [_ w1348]
              frame False {
              }
              frame True {
                n634 = Index Array(array=w1348, index=w1357) -> (element=w1369:waveform(dbl))
                n635 = call-poly <vilib>:"Extract Single Tone Information.vi"("time signal in"=w1369) -> ("detected phase (deg)"=w1352:dbl, "detected frequency"=w1354:dbl)  [unwired: 5 in, 4 out]
                n636 = Format Into String(format string="%.1f (Hz)", w1354) -> (resulting string=w1353:string)  [unwired: 2 in, 1 out]
                n637 = Format Into String(format string="%.0f (°)", w1352) -> (resulting string=w1351:string)  [unwired: 2 in, 1 out]
                n638 = call "Display Synchronous.vi"("Sampling"=w1355, "error in (no error)"=w1356, "phase (°)"=w1352, "frequency (Hz)"=w1354, "Input Waveforms"=w1367) -> ("error out"=w1365:errorcluster, "Output Waveforms"=w1368:waveform(dbl)[])  [unwired: 5 in]
                n639 = call "Display Synchronous.vi"("Sampling"=w1355, "error in (no error)"=w1362, "phase (°)"=w1352, "frequency (Hz)"=w1354, "Input Waveforms"=w1366) -> ("error out"=w1364:errorcluster, "Output Waveforms"=w1363:waveform(dbl)[])  [unwired: 5 in]
                n640 = call "Display Synchronous.vi"("Sampling"=w1355, "error in (no error)"=w1360, "phase (°)"=w1352, "frequency (Hz)"=w1354, "Input Waveforms"=w1361) -> ("error out"=w1359:errorcluster, "Output Waveforms"=w1358:waveform(dbl)[])  [unwired: 5 in]
              }
            }
            "phi (°)" <- w1321
            "f (Hz)" <- w1322
            n641 = local read "X Scale"() -> (w1308:enum16{"time", "samples"})
            n642 = call "Display n or dt.vi"("error in (no error)"=w1310, "X Scale"=w1308, "Input Waveforms"=w1309) -> ("error out"=w1307:errorcluster, "Output Waveforms"=→"REF Graph":waveform(dbl)[])  [unwired: 7 in]
            n643 = call "Display n or dt.vi"("error in (no error)"=w1315, "X Scale"=w1308, "Input Waveforms"=w1314) -> ("error out"=w1338:errorcluster, "Output Waveforms"=w1313:waveform(dbl)[])  [unwired: 7 in]
            n644 = call "Display n or dt.vi"("error in (no error)"=w1312, "X Scale"=w1308, "Input Waveforms"=w1311) -> ("error out"=w1333:errorcluster, "Output Waveforms"=→"AO Graph":waveform(dbl)[])  [unwired: 7 in]
            n645 = local read "Input"() -> (w1336:enum16{"Device", "ADC"})
            n646 = case shown="\"ADC\"" w1336 {
              tunnel: w1313 -> [w1373 w1378]
              tunnel: w1329 -> [_ w1376]
              tunnel: [w1373 w1377] -> w1332
              tunnel: w1338 -> [w1372 w1375]
              tunnel: [w1372 w1374] -> w1334
              frame "Device", Default {
              }
              frame "ADC" {
                n647 = call "Multiply by Gain.vi"("error in (no error)"=w1375, "Gain"=w1376, "WFM in"=w1378) -> ("error out"=w1374:errorcluster, "WFM out"=w1377:waveform(dbl)[])  [unwired: 7 in]
              }
            }
            "AI Graph" <- w1332
            n648 = Merge Errors(w1334, w1333, w1307) -> (w1335:errorcluster)
            n649 = call <vilib>:"Add State(s) to Queue__jki_lib_state_machine.vi"("State(s) in (\"\")"=w1341) -> ("States Out"=w1340:string)  [unwired: 14 in]
          }
          frame "UI: Update AI Waveform Graphs Legends" {
            # "Do not put any code in this frame.\n(It is a separator no-op. You can make a copy of this frame to create a new UI frame)"
            n650 = Unbundle By Name(w1388) -> ("References.Graphs.AI Graph"=w1380:refnum<vi>, "References.Graphs.Sweep AI Graph"=w1379:refnum<vi>, "UI Config.DAQ.Configuration"=w1386:T9)
            n651 = call "Get AI StringsAndValues.vi"("error in (no error)"=w1385, "Configuration.DAQ"=w1386) -> ("error out"=w1383:errorcluster, "Strings"=w1384:string[])  [unwired: 7 in, 1 out]
            n652 = call-poly "Set Legend.vi"("error in (no error)"=w1383, "Plot.Plot Name"=w1384, "WFGraph in"=w1379) -> ("error out"=w1381:errorcluster)  [unwired: 8 in]
            n653 = call-poly "Set Legend.vi"("error in (no error)"=w1383, "Plot.Plot Name"=w1384, "WFGraph in"=w1380) -> ("error out"=w1382:errorcluster)  [unwired: 8 in]
            n654 = Merge Errors(w1382, w1381) -> (w1387:errorcluster)
            n655 = call <vilib>:"Add State(s) to Queue__jki_lib_state_machine.vi"("State(s) in (\"\")"=w1391) -> ("States Out"=w1390:string)  [unwired: 14 in]
          }
          frame "UI: Update AI Waveform Graphs Colors" {
            # "Do not put any code in this frame.\n(It is a separator no-op. You can make a copy of this frame to create a new UI frame)"
            n656 = Unbundle By Name(w1402) -> ("References.Graphs.PS WFGraph"=w1398:refnum<vi>, "References.Graphs.AI Graph"=w1399:refnum<vi>, "References.Graphs.Sweep AI Graph"=w1400:refnum<vi>)
            n657 = call-poly "Set Plot Color.vi"("error in (no error)"=w1393, "WFGraph in"=w1400) -> ("error out"=w1395:errorcluster)  [unwired: 9 in]
            n658 = call-poly "Set Plot Color.vi"("error in (no error)"=w1393, "WFGraph in"=w1399) -> ("error out"=w1396:errorcluster)  [unwired: 9 in]
            n659 = call-poly "Set Plot Color.vi"("error in (no error)"=w1393, "WFGraph (WDT) in"=w1398) -> ("error out"=w1397:errorcluster)  [unwired: 9 in]
            n660 = control-ref of="PS Chart"() -> (w1394:refnum<vi>)
            n661 = call-poly "Set Plot Color.vi"("error in (no error)"=w1393, "PS Chart 2"=w1394) -> ("error out"=w1392:errorcluster)  [unwired: 9 in]
            n662 = Merge Errors(w1392, w1397, w1396, w1395) -> (w1401:errorcluster)
            n663 = call <vilib>:"Add State(s) to Queue__jki_lib_state_machine.vi"("State(s) in (\"\")"=w1405) -> ("States Out"=w1404:string)  [unwired: 14 in]
          }
          frame "UI: Update AO Waveform Graphs Legends" {
            n664 = Unbundle By Name(w1415) -> ("References.Graphs.AO Graph"=w1413:refnum<vi>, "References.Graphs.Sweep AO Graph"=w1412:refnum<vi>, "UI Config.DAQ.Configuration"=w1409:T9)
            n665 = call "Get AO StringsAndValues.vi"("error in (no error)"=w1406, "Configuration.DAQ"=w1409) -> ("error out"=w1407:errorcluster, "Strings"=w1408:string[])  [unwired: 7 in, 1 out]
            n666 = call-poly "Set Legend.vi"("error in (no error)"=w1407, "Plot.Plot Name"=w1408, "WFGraph in"=w1412) -> ("error out"=w1410:errorcluster)  [unwired: 8 in]
            n667 = call-poly "Set Legend.vi"("error in (no error)"=w1407, "Plot.Plot Name"=w1408, "WFGraph in"=w1413) -> ("error out"=w1411:errorcluster)  [unwired: 8 in]
            n668 = Merge Errors(w1411, w1410) -> (w1414:errorcluster)
            n669 = call <vilib>:"Add State(s) to Queue__jki_lib_state_machine.vi"("State(s) in (\"\")"=w1418) -> ("States Out"=w1417:string)  [unwired: 14 in]
          }
          frame "UI: Update REF Waveform Graphs Legends" {
            n670 = Unbundle By Name(w1426) -> ("References.Graphs.REF Graph"=w1424:refnum<vi>, "UI Config.Channels.Cfg_REF"=w1425:T2)
            n671 = call "Get AI REF StringsAndValues.vi"("error in (no error)"=w1420, "Channels.REF"=w1425) -> ("error out"=w1423:errorcluster, "Strings"=w1421:string[])  [unwired: 7 in, 1 out]
            n672 = for {
              tunnel: [w1435] -> w1422 mode=concatenating
              tunnel: w1421 -> [w1430] mode=indexing
              n673 = Concatenate Strings(w1430, " X" ("string")) -> (w1434:string)
              n674 = Concatenate Strings(w1430, " Y" ("string")) -> (w1431:string)
              n675 = Build Array(w1434, w1431) -> (w1435:string[])
            }
            n676 = call-poly "Set Legend.vi"("error in (no error)"=w1423, "Plot.Plot Name"=w1422, "WFGraph in"=w1424) -> ("error out"=w1419:errorcluster)  [unwired: 8 in]
            n677 = call <vilib>:"Add State(s) to Queue__jki_lib_state_machine.vi"("State(s) in (\"\")"=w1429) -> ("States Out"=w1428:string)  [unwired: 14 in]
          }
          frame "UI: Update AO Waveform Graphs Colors" {
            n678 = Unbundle By Name(w1442) -> ("References.Graphs.AO Graph"=w1439:refnum<vi>, "References.Graphs.Sweep AO Graph"=w1440:refnum<vi>)
            n679 = call-poly "Set Plot Color.vi"("error in (no error)"=w1436, "WFGraph in"=w1440) -> ("error out"=w1437:errorcluster)  [unwired: 9 in]
            n680 = call-poly "Set Plot Color.vi"("error in (no error)"=w1436, "WFGraph in"=w1439) -> ("error out"=w1438:errorcluster)  [unwired: 9 in]
            n681 = Merge Errors(w1436, w1438, w1437) -> (w1441:errorcluster)
            n682 = call <vilib>:"Add State(s) to Queue__jki_lib_state_machine.vi"("State(s) in (\"\")"=w1445) -> ("States Out"=w1444:string)  [unwired: 14 in]
          }
          frame "UI: Update REF Waveform Graphs Colors" {
            n683 = Unbundle By Name(w1449) -> ("References.Graphs.REF Graph"=w1448:refnum<vi>)
            n684 = call-poly "Set Plot Color.vi"("error in (no error)"=w1446, "WFGraph in"=w1448) -> ("error out"=w1447:errorcluster)  [unwired: 9 in]
            n685 = call <vilib>:"Add State(s) to Queue__jki_lib_state_machine.vi"("State(s) in (\"\")"=w1452) -> ("States Out"=w1451:string)  [unwired: 14 in]
          }
          frame "UI: Show Hide AO Waveform Graphs" {
            n686 = Unbundle By Name(w1463) -> ("References.Graphs.REF Graph"=w1460:refnum<vi>, "References.Graphs.AO Graph"=w1461:refnum<vi>)
            n687 = local read "Output"() -> (w1459:enum16{"AO", "REF"})
            n688 = Equal?(x=w1459, y=enum16{"Analog Output", "Reference"}."Analog Output" ("Y Axis (Output)")) -> (x = y?=w1454:bool)
            n689 = property on="AO Graph None" class="Bool (strict)"("Visible"=w1454) -> ()  [unwired: 2 in, 2 out]
            n690 = property on="AO Graph All" class="Bool (strict)"("Visible"=w1454) -> ()  [unwired: 2 in, 2 out]
            n691 = property class="WFGraph (strict)"(reference=w1461, "Visible"=w1454) -> (error out=w1457:errorcluster)  [unwired: 1 in, 1 out]
            n692 = Not(x=w1454) -> (.not. x?=w1453:bool)
            n693 = property class="WFGraph (strict)"(reference=w1460, "Visible"=w1453) -> (error out=w1458:errorcluster)  [unwired: 1 in, 1 out]
            n694 = property on="REF Graph None" class="Bool (strict)"("Visible"=w1453) -> ()  [unwired: 2 in, 2 out]
            n695 = property on="REF Graph All" class="Bool (strict)"("Visible"=w1453) -> ()  [unwired: 2 in, 2 out]
            n696 = Merge Errors(w1455, w1458, w1457) -> (w1462:errorcluster)
            n697 = call <vilib>:"Add State(s) to Queue__jki_lib_state_machine.vi"("State(s) in (\"\")"=w1466) -> ("States Out"=w1465:string)  [unwired: 14 in]
          }
          frame "UI: Update Waveform Graph Labels" {
            n698 = Unbundle By Name(w1480) -> ("References.Graphs.REF Graph"=w1474:refnum<vi>, "References.Graphs.AO Graph"=w1478:refnum<vi>, "References.Graphs.AI Graph"=w1479:refnum<vi>)
            n699 = local read "X Scale"() -> (w1467:enum16{"time", "samples"})
            n700 = call "Set AO AI Graph X Axis (WFGraph).vi"("error in (no error)"=w1468, "X Axis"=w1467, "WaveformGraph in"=w1479) -> ("error out"=w1469:errorcluster)  [unwired: 8 in]
            n701 = call "Set AO AI Graph X Axis (WFGraph).vi"("error in (no error)"=w1468, "X Axis"=w1467, "WaveformGraph in"=w1478) -> ("error out"=w1472:errorcluster)  [unwired: 8 in]
            n702 = call "Set AO Graph Y Axis (WFGraph).vi"("error in (no error)"=w1472, "Y Axis (Output)"=enum16{"Analog Output", "Reference"}."Analog Output", "WaveformGraph in"=w1478) -> ("error out"=w1470:errorcluster)  [unwired: 8 in]
            n703 = call "Set AO AI Graph X Axis (WFGraph).vi"("error in (no error)"=w1468, "X Axis"=w1467, "WaveformGraph in"=w1474) -> ("error out"=w1473:errorcluster)  [unwired: 8 in]
            n704 = call "Set AO Graph Y Axis (WFGraph).vi"("error in (no error)"=w1473, "Y Axis (Output)"=enum16{"Analog Output", "Reference"}."Reference", "WaveformGraph in"=w1474) -> ("error out"=w1471:errorcluster)  [unwired: 8 in]
            n705 = Merge Errors(w1471, w1470, w1469) -> (w1475:errorcluster)
            n706 = call <vilib>:"Add State(s) to Queue__jki_lib_state_machine.vi"("State(s) in (\"\")"=w1483) -> ("States Out"=w1482:string)  [unwired: 14 in]
          }
          frame "UI: Init Graph Data" {
            # "UI: Init Graph Data.\n(IInitialize graphs with data before changing their properties)"
            n707 = Unbundle By Name(w1504) -> ("UI Config.DAQ.Configuration"=w1503:T9, "UI Config.Channels.Cfg_REF"=w1502:T2, "UI Config.Plot.visibility.AI"=w1497:bool[], "UI Config.Plot.visibility.AO"=w1496:bool[], "UI Config.Plot.visibility.Lockin"=w1495:bool[])
            n708 = call "Get AI StringsAndValues.vi"("Configuration.DAQ"=w1503) -> ()  [unwired: 8 in, 3 out]
            n709 = call "Get AO StringsAndValues.vi"("Configuration.DAQ"=w1503) -> ()  [unwired: 8 in, 3 out]
            n710 = call "Get AI REF StringsAndValues.vi"("Channels.REF"=w1502) -> ("Strings"=w1487:string[])  [unwired: 8 in, 2 out]
            n711 = Array Size(array=w1487) -> (size(s)=w1485:i32)
            n712 = Array Size(array=w1497) -> (size(s)=w1494:i32)
            n713 = Array Size(array=w1496) -> (size(s)=w1493:i32)
            n714 = Array Size(array=w1495) -> (size(s)=w1491:i32)
            n715 = Get Date/Time In Seconds() -> (seconds since 1Jan1904=w1501:timestamp)
            n716 = Multiply(x=w1485, y=2) -> (x*y=w1484:i32)
            n717 = Bundle By Name("t0"=w1501) -> (w1489:waveform(dbl))  [unwired: 1 in]
            n718 = Initialize Array(w1489, w1484) -> (w1488:waveform(dbl)[])
            n719 = Initialize Array(w1489, w1494) -> (w1500:waveform(dbl)[])
            n720 = Initialize Array(w1489, w1493) -> (w1499:waveform(dbl)[])
            n721 = Initialize Array(w1489, w1491) -> (w1498:waveform(dbl)[])
            n722 = Initialize Array(cluster{"Wavenumber":dbl[], "Data":dbl[]} {"Wavenumber"=[0.0], "Data"=[0.0]} ("Lockin XY"), w1491) -> (w1490:cluster{"Wavenumber":dbl[], "Data":dbl[]}[])
            n723 = local write "REF Graph"(w1488) -> ()
            n724 = local write "AI Graph"(w1500) -> ()
            n725 = local write "AO Graph"(w1499) -> ()
            n726 = local write "Lockin 1"(w1498) -> ()
            n727 = local write "Lockin 2"(w1498) -> ()
            n728 = local write "Lockin XY"(w1490) -> ()
            n729 = call <vilib>:"Add State(s) to Queue__jki_lib_state_machine.vi"("State(s) in (\"\")"=w1508) -> ("States Out"=w1507:string)  [unwired: 14 in]
          }
          frame "UI: Init Graph Legends" {
            # "Do not put any code in this frame.\n(It is a separator no-op. You can make a copy of this frame to create a new UI frame)"
            n730 = Unbundle By Name(w1521) -> ("References.Graphs.AI Graph"=w1520:refnum<vi>, "References.Graphs.AO Graph"=w1519:refnum<vi>, "References.Graphs.REF Graph"=w1518:refnum<vi>, "References.Graphs.Lockin 1"=w1510:refnum<vi>, "References.Graphs.Lockin 2"=w1509:refnum<vi>, "References.Graphs.Lockin XY"=w1517:refnum<vi>, "References.Graphs.Sweep X Graph"=w1516:refnum<vi>, "References.Graphs.Sweep Y Graph"=w1515:refnum<vi>, "References.Graphs.Sweep AI Graph"=w1514:refnum<vi>, "References.Graphs.Sweep AO Graph"=w1513:refnum<vi>, "References.Graphs.PS WFGraph"=w1512:refnum<vi>)  [unwired: 1 out]
            n731 = Build Array(w1520, w1519, w1518, w1510, w1509, w1517, w1516, w1515, w1514, w1513, w1512) -> (w1522:refnum<vi>[])
            n732 = for {
              tunnel: w1522 -> [w1528] mode=indexing
              tunnel: u32 142 ("Legend:Size:Width") -> [w1527]
              n733 = property on="Property Node" class="WFGraph"(reference=w1528, "LegWidth"=w1527) -> ()  [unwired: 1 in, 2 out]
            }
            n734 = call <vilib>:"Add State(s) to Queue__jki_lib_state_machine.vi"("State(s) in (\"\")"=w1526) -> ("States Out"=w1525:string)  [unwired: 14 in]
          }
          frame "UI: Update Lockin Graphs" {
            # "data used in PS"
            n735 = Unbundle By Name(w1536) -> ("clear lockin charts"=w1530:bool, "UI Config.DAQ.cfg.Sampling.Fs.Output"=w1535:dbl, "getAll.Results.Results (Dictionary)"=w1551:cluster{"key":string, "value":dbl[]}[], "UI Config.DAQ.Configuration"=w1550:T9, "UI Config.Amplifers.Gain_AI"=w1549:T17)
            n736 = call "Parse Results (table).vi"("error in (no error)"=w1557, "Input Gain"=w1549, "DAQ Config"=w1550, "Results (Dictionary)"=w1551) -> ("error out"=w1555:errorcluster, "Table"=→"Results":string[][], "Results (Dictionary) out"=w1553:cluster{"key":string, "value":dbl[]}[])  [unwired: 5 in]
            n737 = local read "Display 1"() -> (w1538:T26)
            n738 = local read "Display 2"() -> (w1539:T26)
            n739 = call "Dictionary to Chart.vi"("reset"=w1530, "error in (no error)"=w1555, "Fs.Output (S/s)"=w1535, "Results (Dictionary)"=w1553) -> ("error out"=w1541:errorcluster, "Waveform Graph"=w1533:waveform(dbl)[][], "Results (Dictionary) out"=w1542:cluster{"key":string, "value":dbl[]}[])  [unwired: 5 in]
            n740 = Index Array(array=w1533, index (row) #1=w1538, index (row) #2=w1539) -> (element #1=→"Lockin 1":waveform(dbl)[], element #2=→"Lockin 2":waveform(dbl)[])  [unwired: 2 in]
            n741 = Bundle By Name(cluster=w1536, "clear lockin charts"=FALSE, "Waveform Charts"=w1533) -> (w1537:T65)
            n742 = local read "channel-reference"() -> (w1540:u16)
            n743 = call "Dictionary to XY Graph.vi"("error in (no error)"=w1541, "Results (Dictionary)"=w1542) -> ("error out"=w1547:errorcluster, "XY Graph"=→"Lockin XY":cluster{dbl[], dbl[]}[], "Results (Dictionary) out"=w1548:cluster{"key":string, "value":dbl[]}[])  [unwired: 7 in]
            n744 = call "Dictionary to Indicator.vi"("Results (Dictionary)"=w1548, "AI Channel"=w1540, "error in (no error)"=w1547) -> ("X"=→"X (V)":dbl, "Y"=→"Y (V)":dbl, "R"=→"R (V)":dbl, "Theta"=→"theta (°)":dbl, "Mean"=→"mean (V)":dbl, "error out"=w1556:errorcluster)  [unwired: 7 in]
            n745 = call <vilib>:"Add State(s) to Queue__jki_lib_state_machine.vi"("State(s) in (\"\")"=w1560) -> ("States Out"=w1559:string)  [unwired: 14 in]
          }
          frame "UI: Update Lockin Graphs Legends" {
            n746 = Unbundle By Name(w1569) -> ("References.Graphs.Sweep X Graph"=w1581:refnum<vi>, "References.Graphs.Sweep Y Graph"=w1580:refnum<vi>, "References.Graphs.Lockin XY"=w1579:refnum<vi>, "References.Graphs.Lockin 2"=w1578:refnum<vi>, "References.Graphs.Lockin 1"=w1576:refnum<vi>)
            n747 = Unbundle By Name(w1569) -> ("UI Config.DAQ.Configuration"=w1571:T9, "UI Config.Channels.Cfg_REF"=w1570:T2)
            n748 = call "Get AI REF StringsAndValues.vi"("error in (no error)"=w1564, "Channels.REF"=w1570) -> ("error out"=w1565:errorcluster, "Strings"=w1567:string[])  [unwired: 7 in, 1 out]
            n749 = call "Get AI StringsAndValues.vi"("error in (no error)"=w1565, "Configuration.DAQ"=w1571) -> ("error out"=w1563:errorcluster, "Strings"=w1568:string[])  [unwired: 7 in, 1 out]
            n750 = call <vilib>:"Space Constant.vi"() -> ("String"=w1562:string)
            n751 = for {
              tunnel: w1568 -> [w1587]
              tunnel: w1567 -> [w1588] mode=indexing
              tunnel: [w1586] -> w1566 mode=concatenating
              tunnel: w1562 -> [w1585]
              n752 = for {
                tunnel: w1588 -> [w1591]
                tunnel: w1587 -> [w1590] mode=indexing
                tunnel: [w1592] -> w1586 mode=indexing
                tunnel: w1585 -> [w1589]
                n753 = Concatenate Strings(w1590, w1589, w1591) -> (w1592:string)
              }
            }
            n754 = call-poly "Set Legend.vi"("error in (no error)"=w1563, "Plot.Plot Name"=w1566, "WFGraph in"=w1576) -> ("error out"=w1572:errorcluster)  [unwired: 8 in]
            n755 = call-poly "Set Legend.vi"("error in (no error)"=w1563, "Plot.Plot Name"=w1566, "WFGraph in"=w1578) -> ("error out"=w1573:errorcluster)  [unwired: 8 in]
            n756 = call-poly "Set Legend.vi"("error in (no error)"=w1563, "Plot.Plot Name"=w1566, "XYGraph in"=w1579) -> ("error out"=w1574:errorcluster)  [unwired: 8 in]
            n757 = call-poly "Set Legend.vi"("error in (no error)"=w1563, "Plot.Plot Name"=w1566, "WFGraph in"=w1580) -> ("error out"=w1575:errorcluster)  [unwired: 8 in]
            n758 = call-poly "Set Legend.vi"("error in (no error)"=w1563, "Plot.Plot Name"=w1566, "WFGraph in"=w1581) -> ("error out"=w1561:errorcluster)  [unwired: 8 in]
            n759 = Merge Errors(w1561, w1575, w1574, w1573, w1572) -> (w1577:errorcluster)
            n760 = call <vilib>:"Add State(s) to Queue__jki_lib_state_machine.vi"("State(s) in (\"\")"=w1584) -> ("States Out"=w1583:string)  [unwired: 14 in]
          }
          frame "UI: Update Lockin Graphs Colors" {
            n761 = Unbundle By Name(w1605) -> ("References.Graphs.Sweep X Graph"=w1604:refnum<vi>, "References.Graphs.Sweep Y Graph"=w1603:refnum<vi>, "References.Graphs.Lockin XY"=w1593:refnum<vi>, "References.Graphs.Lockin 2"=w1602:refnum<vi>, "References.Graphs.Lockin 1"=w1601:refnum<vi>)
            n762 = call-poly "Set Plot Color.vi"("error in (no error)"=w1594, "WFGraph in"=w1601) -> ("error out"=w1595:errorcluster)  [unwired: 9 in]
            n763 = call-poly "Set Plot Color.vi"("error in (no error)"=w1594, "WFGraph in"=w1602) -> ("error out"=w1596:errorcluster)  [unwired: 9 in]
            n764 = call-poly "Set Plot Color.vi"("error in (no error)"=w1594, "XYGraph in"=w1593) -> ("error out"=w1597:errorcluster)  [unwired: 9 in]
            n765 = call-poly "Set Plot Color.vi"("error in (no error)"=w1594, "WFGraph in"=w1603) -> ("error out"=w1598:errorcluster)  [unwired: 9 in]
            n766 = call-poly "Set Plot Color.vi"("error in (no error)"=w1594, "WFGraph in"=w1604) -> ("error out"=w1599:errorcluster)  [unwired: 9 in]
            n767 = while {
              tunnel: w1593 -> [w1612]
              i -> [w1610]
              stop <- w1611 stop-if-true
              n768 = property on="Property Node" class="XYGraph (strict)"(reference=w1612, "Active Plot"=w1610, "Plot.Point Style"=u8 1) -> (error out=w1611:errorcluster)  [unwired: 1 in, 1 out]
            }
            n769 = Merge Errors(w1599, w1598, w1597, w1596, w1595) -> (w1600:errorcluster)
            n770 = call <vilib>:"Add State(s) to Queue__jki_lib_state_machine.vi"("State(s) in (\"\")"=w1608) -> ("States Out"=w1607:string)  [unwired: 14 in]
          }
          frame "UI: Update Lockin Graph Range" {
            # "xy"
            # "2"
            # "1"
            # "Do not put any code in this frame.\n(It is a separator no-op. You can make a copy of this frame to create a new UI frame)"
            n771 = Unbundle By Name(w1620) -> ("References.Graphs.Lockin 1"=w1617:refnum<vi>, "References.Graphs.Lockin 2"=w1616:refnum<vi>, "References.Graphs.Lockin XY"=w1615:refnum<vi>)
            n772 = Negate(x="X/R Range") -> (-x=w1621:dbl)
            n773 = Negate(x="Y/Theta Range") -> (-x=w1622:dbl)
            n774 = Negate(x="XY Range") -> (-x=w1614:dbl)
            n775 = property on="Property Node" class="WFGraph (strict)"(reference=w1617, "YScale.Maximum"="X/R Range", "YScale.Minimum"=w1621) -> ()  [unwired: 1 in, 2 out]
            n776 = property on="Property Node" class="WFGraph (strict)"(reference=w1616, "YScale.Maximum"="Y/Theta Range", "YScale.Minimum"=w1622) -> ()  [unwired: 1 in, 2 out]
            n777 = property on="Property Node" class="XYGraph (strict)"(reference=w1615, "XScale.Maximum"="XY Range", "YScale.Maximum"="XY Range", "XScale.Minimum"=w1614, "YScale.Minimum"=w1614) -> ()  [unwired: 1 in, 2 out]
            n778 = call <vilib>:"Add State(s) to Queue__jki_lib_state_machine.vi"("State(s) in (\"\")"=w1626) -> ("States Out"=w1625:string)  [unwired: 14 in]
          }
          frame "UI: Update Lockin Graph Labels" {
            n779 = local read "Display 1"() -> (w1633:T26)
            n780 = local read "Display 2"() -> (w1627:T26)
            n781 = Unbundle By Name(w1629) -> ("References.Graphs.Lockin 1"=w1631:refnum<vi>, "References.Graphs.Lockin 2"=w1630:refnum<vi>)
            n782 = case shown="\"Mean\"" w1633 {
              tunnel: ["Lockin X (A or V)" "Lockin Y (A or V)" "R (A or V)" "Theta (°)" "Mean (A or V)"] -> w1632
              frame "X", Default {
              }
              frame "Y" {
              }
              frame "R" {
              }
              frame "Theta" {
              }
              frame "Mean" {
              }
            }
            n783 = case shown="\"Mean\"" w1627 {
              tunnel: ["Lockin X (A or V)" "Lockin Y (A or V)" "R (A or V)" "Theta (°)" "Mean (A or V)"] -> w1628
              frame "X", Default {
              }
              frame "Y" {
              }
              frame "R" {
              }
              frame "Theta" {
              }
              frame "Mean" {
              }
            }
            n784 = property on="Property Node" class="WFGraph (strict)"(reference=w1631, "YScale.NameLbl.Text"=w1632) -> ()  [unwired: 1 in, 2 out]
            n785 = property on="Property Node" class="WFGraph (strict)"(reference=w1630, "YScale.NameLbl.Text"=w1628) -> ()  [unwired: 1 in, 2 out]
            n786 = call <vilib>:"Add State(s) to Queue__jki_lib_state_machine.vi"("State(s) in (\"\")"=w1637) -> ("States Out"=w1636:string)  [unwired: 14 in]
          }
          frame "UI: Update Sweep Graphs" {
            # "UI: Update Sweep Graphs.\n()"
            n787 = Unbundle By Name(w1654) -> ("getAll.SweepWaveforms.AO"=w1650:waveform(dbl)[], "getAll.SweepWaveforms.AI"=w1653:waveform(dbl)[], "getAll.SweepWaveforms.X"=w1652:waveform(dbl)[], "getAll.SweepWaveforms.Y"=w1651:waveform(dbl)[])
            n788 = Empty Array?(array=w1650) -> (empty?=w1649:bool)
            n789 = Not(x=w1649) -> (.not. x?=w1648:bool)
            n790 = case shown="True" w1648 {
              tunnel: w1653 -> [_ w1662]
              tunnel: w1652 -> [_ w1661]
              tunnel: w1651 -> [_ w1660]
              tunnel: w1650 -> [_ w1659]
              frame False {
              }
              frame True {
                "Sweep X" <- w1661
                "Sweep AO" <- w1659
                "Sweep AI" <- w1662
                "Sweep Y" <- w1660
              }
            }
            n791 = call <vilib>:"Add State(s) to Queue__jki_lib_state_machine.vi"("State(s) in (\"\")"=w1658) -> ("States Out"=w1657:string)  [unwired: 14 in]
          }
          frame "UI: Update Sweep Timer" {
            # "Do not put any code in this frame.\n(It is a separator no-op. You can make a copy of this frame to create a new UI frame)"
            n792 = local read "Sweep Time (s)"() -> (w1666:dbl)
            n793 = local read "Initial Wait (s)"() -> (w1665:dbl)
            n794 = Unbundle By Name(w1664) -> ("DAQ state"=w1663:T33)
            n795 = case shown="\"sweeping\"" w1663 {
              tunnel: [0.0 w1676] -> w1667
              tunnel: w1666 -> [_ w1674]
              tunnel: w1665 -> [_ w1673]
              frame Default {
              }
              frame "sweeping" {
                # "some overhead"
                n796 = call <userlib>:"MGI Milliseconds Since Last Reset.vi"() -> ("ms"=w1680:u32)  [unwired: 6 in, 1 out]
                n797 = Divide(x=w1680, y=u32 1000) -> (x/y=w1678:dbl)
                n798 = Negate(x=w1678) -> (-x=w1677:dbl)
                n799 = Compound Arithmetic op=ADD(2.0 ("value"), w1673, w1674, w1677) -> (w1676:dbl)
              }
            }
            n800 = local write "Sweep Timer (s)"(w1667) -> ()
            n801 = call <vilib>:"Add State(s) to Queue__jki_lib_state_machine.vi"("State(s) in (\"\")"=w1671) -> ("States Out"=w1670:string)  [unwired: 14 in]
          }
          frame "UI: Update Sweep Config" {
            # "UI: Update Sweep Config\n(Called by <DAQ Public Events.getSweepChannels>: User Event)"
            n802 = Unbundle By Name(w1687) -> ("UI Config.Sweep"=w1683:T55)
            n803 = Unbundle By Name(w1683) -> ("sweepTime"=w1685:dbl, "initialWaitTime"=w1686:dbl, "returnToStart"=w1684:bool, "sweepChannels"=w1681:T20)
            n804 = for {
              tunnel: w1681 -> [w1695] mode=indexing
              tunnel: [w1692] -> w1682 mode=indexing
              n805 = Unbundle By Name(w1695) -> ("Channel"=w1694:u16, "Table"=w1693:dbl[])
              n806 = Bundle("Channel"=w1694, "Table"=w1693) -> (w1692:cluster{"Channel":u16, "Table":dbl[]})  [unwired: 1 in]
            }
            n807 = local write "Sweep Time (s)"(w1685) -> ()
            n808 = local write "Initial Wait (s)"(w1686) -> ()
            n809 = local write "Return to Start?"(w1684) -> ()
            n810 = local write "Sweep Channels"(w1681) -> ()
            n811 = local write "Sweep Pattern"(w1682) -> ()
            n812 = call <vilib>:"Add State(s) to Queue__jki_lib_state_machine.vi"("State(s) in (\"\")"=w1691) -> ("States Out"=w1690:string)  [unwired: 14 in]
          }
          frame "UI: Initialize PS Graph" {
            # "Do not put any code in this frame.\n(It is a separator no-op. You can make a copy of this frame to create a new UI frame)"
            n813 = Unbundle By Name(w1701) -> ("UI Config.Plot.visibility.AI"=w1699:bool[])
            n814 = Array Size(array=w1699) -> (size(s)=w1696:i32)
            n815 = Initialize Array(cluster{"f0":dbl, "df":dbl, "magnitude":dbl[]} {"f0"=0.0, "df"=1.0, "magnitude"=[0.001]} ("power spectrum"), w1696) -> (w1697:cluster{"f0":dbl, "df":dbl, "magnitude":dbl[]}[])
            n816 = local write "PS Waveform"(w1697) -> ()
            n817 = call <vilib>:"Add State(s) to Queue__jki_lib_state_machine.vi"("State(s) in (\"\")"=w1704) -> ("States Out"=w1703:string)  [unwired: 14 in]
          }
          frame "UI: Update PS Graph Labels" {
            n818 = local read "export mode"() -> (w1708:u16)
            n819 = local read "PS Display"() -> (w1706:enum16{"AO", "AI", "X", "Y", "R", "Theta"})
            n820 = case shown="0, Default" w1708 {
              tunnel: ["%s power spectrum (dB( ))" ("Y Scale.Name Label.Text") "%s power strectral density (dB( )/Hz)" ("Y Scale.Name Label.Text")] -> w1707
              frame 0, Default {
              }
              frame 1 {
              }
            }
            n821 = Unbundle By Name(w1709) -> ("References.Graphs.PS WFGraph"=w1710:refnum<vi>)
            n822 = Format Into String(format string=w1707, w1706) -> (resulting string=w1705:string)  [unwired: 2 in, 1 out]
            n823 = property on="Property Node" class="WFGraph (strict)"(reference=w1710, "YScale.NameLbl.Text"=w1705) -> ()  [unwired: 1 in, 2 out]
            n824 = call <vilib>:"Add State(s) to Queue__jki_lib_state_machine.vi"("State(s) in (\"\")"=w1714) -> ("States Out"=w1713:string)  [unwired: 14 in]
          }
          frame "UI: Update PS Graph Legend" {
            # "UI: Update PS Graph Legend.\n()"
            n825 = local read "PS Display"() -> (w1723:enum16{"AO", "AI", "X", "Y", "R", "Theta"})
            n826 = Unbundle By Name(w1722) -> ("References.Graphs.PS WFGraph"=w1719:refnum<vi>)
            n827 = case shown="\"X\"..\"Theta\"" w1723 {
              tunnel: w1722 -> [w1730 w1736 w1742]
              tunnel: [w1731 w1734 w1738] -> w1720
              tunnel: [w1728 w1732 w1739] -> w1721
              tunnel: w1717 -> [w1727 w1733 w1741]
              frame "AO" {
                n828 = Unbundle By Name(w1730) -> ("UI Config.DAQ.Configuration"=w1729:T9)
                n829 = call "Get AO StringsAndValues.vi"("error in (no error)"=w1727, "Configuration.DAQ"=w1729) -> ("error out"=w1728:errorcluster, "Strings"=w1731:string[])  [unwired: 7 in, 1 out]
              }
              frame "AI" {
                n830 = Unbundle By Name(w1736) -> ("UI Config.DAQ.Configuration"=w1735:T9)
                n831 = call "Get AI StringsAndValues.vi"("error in (no error)"=w1733, "Configuration.DAQ"=w1735) -> ("error out"=w1732:errorcluster, "Strings"=w1734:string[])  [unwired: 7 in, 1 out]
              }
              frame "X".."Theta" {
                n832 = Unbundle By Name(w1742) -> ("UI Config.DAQ.Configuration"=w1743:T9, "UI Config.Channels.Cfg_REF"=w1744:T2)
                n833 = call "Get AI REF StringsAndValues.vi"("error in (no error)"=w1741, "Channels.REF"=w1744) -> ("error out"=w1740:errorcluster, "Strings"=w1746:string[])  [unwired: 7 in, 1 out]
                n834 = call "Get AI StringsAndValues.vi"("error in (no error)"=w1740, "Configuration.DAQ"=w1743) -> ("error out"=w1739:errorcluster, "Strings"=w1745:string[])  [unwired: 7 in, 1 out]
                n835 = call <vilib>:"Space Constant.vi"() -> ("String"=w1737:string)
                n836 = for {
                  tunnel: w1745 -> [w1749]
                  tunnel: w1746 -> [w1750] mode=indexing
                  tunnel: [w1748] -> w1738 mode=concatenating
                  tunnel: w1737 -> [w1747]
                  n837 = for {
                    tunnel: w1750 -> [w1753]
                    tunnel: w1749 -> [w1752] mode=indexing
                    tunnel: [w1754] -> w1748 mode=indexing
                    tunnel: w1747 -> [w1751]
                    n838 = Concatenate Strings(w1752, w1751, w1753) -> (w1754:string)
                  }
                }
              }
            }
            n839 = call-poly "Set Legend.vi"("error in (no error)"=w1721, "Plot.Plot Name"=w1720, "WFGraph (WDT) in"=w1719) -> ("error out"=w1718:errorcluster)  [unwired: 8 in]
            n840 = call <vilib>:"Add State(s) to Queue__jki_lib_state_machine.vi"("State(s) in (\"\")"=w1726) -> ("States Out"=w1725:string)  [unwired: 14 in]
          }
          frame "UI: Update Channel Ring" {
            # "UI: Update Channel Ring.\n()"
            n841 = Unbundle By Name(w1762) -> ("getAll.Results.Results (Dictionary)"=w1758:cluster{"key":string, "value":dbl[]}[])
            n842 = local read "channel-reference"() -> (w1757:u16)
            n843 = call "Dictionary to Plot Names.vi"("error in (no error)"=w1760, "Results (Dictionary)"=w1758) -> ("error out"=w1761:errorcluster, "Plot Names"=w1759:string[])  [unwired: 7 in, 1 out]
            n844 = property on="channel-reference" class="Ring (strict)"(error in=w1761, "Strings []"=w1759, "Value"=w1757) -> (error out=w1756:errorcluster)  [unwired: 1 in, 1 out]
            n845 = case shown="No Error" w1756 {
              selector: w1756 -> [w1766 _]
              tunnel: [w1766 _] -> w1755
              frame No Error {
              }
              frame Error {
                n846 = local write "channel-reference"(0) -> ()
              }
            }
            n847 = call <vilib>:"Add State(s) to Queue__jki_lib_state_machine.vi"("State(s) in (\"\")"=w1765) -> ("States Out"=w1764:string)  [unwired: 14 in]
          }
          frame "UI: Update AI REF Channel Ring" {
            # "update AI Ref Channel ring"
            # "Do not put any code in this frame.\n(It is a separator no-op. You can make a copy of this frame to create a new UI frame)"
            n848 = Unbundle By Name(w1771) -> ("UI Config.Channels.Cfg_REF"=w1770:T2)
            n849 = call "Get REF StringsAndValues.vi"("error in (no error)"=w1769, "Channels.REF"=w1770) -> ("error out"=w1773:errorcluster, "REF Strings and Values"=w1772:cluster{string, i32}[])  [unwired: 8 in]
            n850 = property on="reference channel" class="Ring (strict)"(error in=w1773, "StringsAndValues[]"=w1772) -> (error out=w1768:errorcluster)  [unwired: 1 in, 1 out]
            n851 = call <vilib>:"Add State(s) to Queue__jki_lib_state_machine.vi"("State(s) in (\"\")"=w1776) -> ("States Out"=w1775:string)  [unwired: 14 in]
          }
          frame "UI: Sync AI Ref Array" {
            n852 = Scan From String(input string=w1783, default 1=0 ("index")) -> (output 1=w1780:i32)  [unwired: 3 in, 3 out]
            n853 = local read "AI Channels"() -> (w1779:T4)
            n854 = Index Array(array=w1779, index=w1780) -> (element=w1785:T5)
            n855 = Array Size(array=w1779) -> (size(s)=w1778:i32)
            n856 = Unbundle By Name(w1785) -> ("reference index"=w1784:i32)
            n857 = for {
              N: w1778 -> [_]
              tunnel: w1784 -> [w1795]
              shift-right: [w1792] -> w1781
              shift-left: w1779 -> [w1794]
              i -> [w1793]
              n858 = in-place {
                in-place-border: w1795 -> [w1798]
                n859 = in-place-array #1(w1794, w1793) -> (w1797:T5)
                n860 = Bundle By Name(cluster=w1797, "reference index"=w1798) -> (w1796:T5)
                n861 = in-place-array #1(w1796) -> (w1792:T4)  [unwired: 1 out]
              }
            }
            n862 = control-ref of="References"() -> (w1777:refnum<vi>)
            n863 = Build Array(w1784) -> (w1786:i32[])
            n864 = property on="Property Node" class="Arr (strict)"(reference=w1777, "Index Values"=w1786) -> ()  [unwired: 1 in, 2 out]
            n865 = local write "AI Channels"(w1781) -> ()
            n866 = call <vilib>:"Add State(s) to Queue__jki_lib_state_machine.vi"("State(s) in (\"\")"=w1791) -> ("States Out"=w1790:string)  [unwired: 14 in]
          }
          frame "UI: Remove Unused References" {
            # "update Ch.AI after removing\nunused Ch.REF"
            # "Do not put any code in this frame.\n(It is a separator no-op. You can make a copy of this frame to create a new UI frame)"
            n867 = Unbundle By Name(w1804) -> ("UI Config.Channels.Cfg_AI"=w1803:T4, "UI Config.Channels.Cfg_REF"=w1802:T2)
            n868 = call "Remove Unused References.vi"("error in (no error)"=w1800, "Channels.REF"=w1802, "Channels.AI"=w1803) -> ("error out"=w1801:errorcluster, "Channels.AI out"=w1799:T4)  [unwired: 7 in]
            n869 = local write "AI Channels"(w1799) -> ()
            n870 = call <vilib>:"Add State(s) to Queue__jki_lib_state_machine.vi"("State(s) in (\"\")"=w1807) -> ("States Out"=w1806:string)  [unwired: 14 in]
          }
          frame "UI: Update AI REF Channels" {
            # "UI: Update AI REF Channels\n(enable/disable demodulation channels)"
            n871 = Unbundle By Name(w1810) -> ("UI Config.Channels.Cfg_AI"=w1814:T4, "UI Config.Channels.Cfg_REF"=w1808:T2)
            n872 = case shown="\"All 1\"" w1809 {
              tunnel: [w1819 i32[] [0] ("References")] -> w1813
              tunnel: w1808 -> [w1820 _]
              frame "All 1" {
                n873 = for {
                  tunnel: w1820 -> [w1823] mode=indexing
                  tunnel: [w1822] -> w1819 mode=indexing if=w1821
                  n874 = Unbundle By Name(w1823) -> ("Channel"=w1822:i32, "Enable?"=w1821:bool)
                }
              }
              frame "Disable", Default {
              }
            }
            n875 = for {
              tunnel: w1814 -> [w1827] mode=indexing
              tunnel: [w1826] -> w1811 mode=indexing
              tunnel: w1813 -> [w1825]
              n876 = Bundle By Name(cluster=w1827, "References"=w1825) -> (w1826:T5)
            }
            n877 = Bundle By Name(cluster=w1810, "UI Config.Channels.Cfg_AI"=w1811) -> (w1812:T65)
            n878 = local write "AI Channels"(w1811) -> ()
            n879 = call <vilib>:"Add State(s) to Queue__jki_lib_state_machine.vi"("State(s) in (\"\")"=w1818) -> ("States Out"=w1817:string)  [unwired: 14 in]
          }
          frame "UI: Update Sampling Status" {
            # "Do not put any code in this frame.\n(It is a separator no-op. You can make a copy of this frame to create a new UI frame)"
            n880 = Unbundle By Name(w1832) -> ("getAll.Waveforms.AI"=w1831:waveform(dbl)[])
            n881 = call <userlib>:"MGI Milliseconds Since Last Call.vi"() -> ("ms"=w1839:u32)  [unwired: 6 in, 1 out]
            "Wfm Refresh Time (ms)" <- w1839
            n882 = Index Array(array=w1831) -> (element=w1845:waveform(dbl))  [unwired: 1 in]
            n883 = call-poly <vilib>:"Waveform Duration.vi"("error in (no error)"=w1829, "waveform in"=w1845) -> ("error out"=w1830:errorcluster, "duration"=w1844:dbl)  [unwired: 7 in, 1 out]
            n884 = Multiply(x=w1844, y=1000.0) -> (x*y=w1843:dbl)
            n885 = Multiply(x=w1843, y=2.0) -> (x*y=w1842:dbl)
            n886 = Less?(x=w1839, y=w1842) -> (x < y?=w1841:bool)
            n887 = Select(t=u32 6618880, s=w1841, f=u32 16711680) -> (s? t:f=→"Sampling Status":u32)
            n888 = Select(t="Good", s=w1841, f="#s/Fs: too small!") -> (s? t:f=→"Sampling Status":string)
            n889 = call <vilib>:"Add State(s) to Queue__jki_lib_state_machine.vi"("State(s) in (\"\")"=w1848) -> ("States Out"=w1847:string)  [unwired: 14 in]
          }
          frame "---------- Macro ----------" {
            # "Do not put any code in this frame.\n(It is a separator no-op. You can make a copy of this frame to create a new Macro frame)"
            n890 = call <vilib>:"Add State(s) to Queue__jki_lib_state_machine.vi"("State(s) in (\"\")"=w1853) -> ("States Out"=w1852:string)  [unwired: 14 in]
          }
          frame "Macro: Initialize" {
            # "Initialization Macro\n(This is called once, when the VI starts)"
            n891 = call <vilib>:"Add State(s) to Queue__jki_lib_state_machine.vi"("State(s) in Front (\"\")"="Data: Initialize\nInitialize Core Data\nEvents: Register", "State(s) in (\"\")"="") -> ("States Out"=w1854:string)  [unwired: 13 in]
            n892 = call <vilib>:"Add State(s) to Queue__jki_lib_state_machine.vi"("State(s) in Front (\"\")"=w1854, "State(s) in (\"\")"="Process: Sync", "State(s) at Back (\"\")"="UI: Initialize\nMacro: Initialize UI Before Open\nUI: Front Panel State >> Open\nMacro: Initialize UI After Open\nData: Wait >> 500\nMacro: Initialize III") -> ("States Out"=w1858:string)  [unwired: 12 in]
            n893 = call <vilib>:"Add State(s) to Queue__jki_lib_state_machine.vi"("State(s) in Front (\"\")"=w1858, "State(s) in (\"\")"=w1864) -> ("States Out"=w1863:string)  [unwired: 13 in]
          }
          frame "Macro: Post Error Handling" {
            # "Clear Last Error?"
            # "Do not put any code in this frame.\n(It is a separator no-op. You can make a copy of this frame to create a new Macro frame)"
            n894 = Unbundle By Name(w1866) -> ("Core.Last Error.remaining states"=w1868:string, "Core.Shutdown?"=w1869:bool)
            n895 = Unbundle By Name(w1866) -> ("Core.Last Error.error"=w1872:errorcluster)
            n896 = case shown="False" FALSE {
              tunnel: w1872 -> [w1880 _]
              tunnel: [w1880 _] -> w1871
              frame False {
              }
              frame True {
              }
            }
            n897 = case shown="True" w1869 {
              tunnel: w1868 -> [w1877 w1879]
              tunnel: [w1877 w1878] -> w1865
              frame False {
                # "These are the remaining states (at the moment the error occured). States can be altered according to business logic."
                # "NOT SHUTTING DOWN"
              }
              frame True {
                # "Developer can decide to alter the states but should be aware that during the shutdown process, there are certain states that must be run for the SMO to properly shut itself (and this process) down. As such, one can add states to perform additional clean-ups, but should append the remaining state to be executed."
                # "SHUTTING DOWN"
                n898 = call <vilib>:"Add State(s) to Queue__jki_lib_state_machine.vi"("State(s) in (\"\")"=w1879) -> ("States Out"=w1878:string)  [unwired: 14 in]
              }
            }
            n899 = Bundle By Name(cluster=w1866, "Core.Last Error.error"=w1871) -> (w1867:T65)
            n900 = call <vilib>:"Add State(s) to Queue__jki_lib_state_machine.vi"("State(s) in Front (\"\")"=w1865, "State(s) in (\"\")"=w1876) -> ("States Out"=w1875:string)  [unwired: 13 in]
          }
          frame "Macro: Initialize UI Before Open" {
            # "Initialize UI\n(This is called after UI: Initialize and before UI: Front Panel State >> Open)"
            n901 = local write "Show DAQ UI"(FALSE ("Show UI")) -> ()
            n902 = call <vilib>:"Add State(s) to Queue__jki_lib_state_machine.vi"("State(s) in Front (\"\")"="UI: Cursor Set >> Busy\nUI: Defer Panel Updates >> TRUE\n\nData: Initialize Control References\nData: Initialize Graph References\n\nUI: Reinit To Default\nUI: Disable Buttons\n\nConfiguration: Initialize\nConfiguration: Read File\nUI: Cluster to UI\nUI: Cluster to UI 2\nUI: Init Graph Data\nUI: Init Graph Legends\nUI: Update PS Graph Legend\nUI: Update Waveform Graph Labels\n\nUI: Defer Panel Updates >> FALSE" ("State(s) in Front (\"\")"), "State(s) in (\"\")"=w1887) -> ("States Out"=w1886:string)  [unwired: 13 in]
          }
          frame "Macro: Initialize UI After Open" {
            # "Initialize UI\n(This is called after UI: Initialize and before UI: Front Panel State >> Open)"
            n903 = Format Into String(format string="UI: Defer Panel Updates >> TRUE\nUI: Set Left Tab >> %s\nUI: Set Right Tab >> %s\nAction: IDN\nUI: Defer Panel Updates >> FALSE\nUI: Cursor Set >> Idle" ("State(s) in Front (\"\")"), T1."Status" ("Left Tab"), T25."AO/AI Graphs" ("Right Tab")) -> (resulting string=w1890:string)  [unwired: 2 in, 1 out]
            n904 = call <vilib>:"Add State(s) to Queue__jki_lib_state_machine.vi"("State(s) in Front (\"\")"=w1890, "State(s) in (\"\")"=w1896) -> ("States Out"=w1895:string)  [unwired: 13 in]
          }
          frame "Macro: Initialize III" {
            # "Initialize UI\n(This is called after UI: Initialize and before UI: Front Panel State >> Open)"
            n905 = Format Into String(format string="UI: Cursor Set >> Busy\n\nMacro: Initialize DAQ\nIdle\nMacro: Initialize Waveform Graphs\nMacro: Initialize Lockin Graphs\n\nIdle\nUI: Defer Panel Updates >> TRUE\nUI: Enable Buttons\nUI: Init Scroll Bars\nUI: Set Left Tab >> %s\nUI: Set Right Tab >> %s\nUI: Defer Panel Updates >> FALSE\n\nUI: Cursor Set >> Idle" ("State(s) in Front (\"\")"), T1."AO/AI/REF" ("Left Tab"), T25."AO/AI Graphs" ("Right Tab")) -> (resulting string=w1899:string)  [unwired: 2 in, 1 out]
            n906 = call <vilib>:"Add State(s) to Queue__jki_lib_state_machine.vi"("State(s) in Front (\"\")"=w1899, "State(s) in (\"\")"=w1905) -> ("States Out"=w1904:string)  [unwired: 13 in]
          }
          frame "Macro: Initialize DAQ" {
            # "Action: State >> reset\n//Action: Offset"
            n907 = call <vilib>:"Delimited String to 1D String Array.vi"("delimiter"="\n", "delimited string"="Action: AI Channels\nAction: AO Channels\nAction: REF Channels\nAction: DAQ Config\nAction: Sampling\nAction: Sampling Fs Mode\nAction: Sampling Fs Multiplier\nAction: Sampling Fs Output\nAction: Sampling Refresh Rate\nAction: Sampling Decimation Pre DSP\nAction: Sampling Decimation Post DSP\nAction: AI Simulate Mode\nAction: Sweep\nAction: Limit Amplitude\nAction: Limit DC\nAction: Link Frequencies\nAction: Duty Cycle\nAction: PreFilter\nAction: Input Gain\nAction: Output Gain\nAction: Offset Mode >> Remove\nAction: Log Configuration" ("State(s) in Front (\"\")")) -> ("string array"=w1906:string[])  [unwired: 9 in]
            n908 = Array Size(array=w1906) -> (size(s)=w1913:i32)
            n909 = Initialize Array("Action: Command\nData: Wait >> 25\n//Idle", w1913) -> (w1912:string[])
            n910 = Interleave 1D Arrays(w1906, w1912) -> (w1907:string[])
            n911 = call <vilib>:"1D String Array to Delimited String.vi"("delimiter"="\n", "string array"=w1907) -> ("delimited string"=w1911:string)  [unwired: 9 in]
            n912 = call <vilib>:"Add State(s) to Queue__jki_lib_state_machine.vi"("State(s) in Front (\"\")"=w1911, "State(s) in (\"\")"=w1919) -> ("States Out"=w1918:string)  [unwired: 13 in]
          }
          frame "Macro: Initialize Waveform Graphs" {
            n913 = call <vilib>:"Add State(s) to Queue__jki_lib_state_machine.vi"("State(s) in Front (\"\")"="UI: Defer Panel Updates >> TRUE\n\nUI: Update Waveform Graphs\nUI: Update Sweep Graphs\n\nUI: Update AI REF Channel Ring\n\nUI: Update AI Waveform Graphs Legends\nUI: Update AI Waveform Graphs Colors\nUI: Update AO Waveform Graphs Legends\nUI: Update AO Waveform Graphs Colors\nUI: Update REF Waveform Graphs Legends\nUI: Update REF Waveform Graphs Colors\n\nUI: Set Plot Visibility //from UI cluster\nUI: Sync AI Plot Visibility\nUI: Sync AO Plot Visibility\nUI: Show Hide AO Waveform Graphs\nUI: Initialize PS Graph\nUI: Update PS Graph Labels\n\nUI: Defer Panel Updates >> FALSE" ("State(s) in Front (\"\")"), "State(s) in (\"\")"=w1925) -> ("States Out"=w1924:string)  [unwired: 13 in]
          }
          frame "Macro: Initialize Lockin Graphs" {
            n914 = call <vilib>:"Add State(s) to Queue__jki_lib_state_machine.vi"("State(s) in Front (\"\")"="UI: Defer Panel Updates >> TRUE\n\nUI: Update Lockin Graphs\n\nUI: Update Channel Ring\nUI: Update Lockin Graph Labels\nUI: Update Lockin Graphs Legends\nUI: Update Lockin Graphs Colors\n\nUI: Sync Lockin Plot Visibility\n\nUI: Defer Panel Updates >> FALSE" ("State(s) in Front (\"\")"), "State(s) in (\"\")"=w1931) -> ("States Out"=w1930:string)  [unwired: 13 in]
          }
          frame "Macro: Update Waveform Graphs" {
            n915 = local read "Right Tab"() -> (w1937:T25)
            n916 = case shown="\"PS\"" w1937 {
              tunnel: ["UI: Update Waveform Graphs" ("State(s) in Front (\"\")") "Action: Power Spectrum" ("State(s) in Front (\"\")") "" ("State(s) in Front (\"\")")] -> w1935
              frame "AO/AI Graphs" {
              }
              frame "PS" {
              }
              frame Default {
              }
            }
            n917 = call <vilib>:"Add State(s) to Queue__jki_lib_state_machine.vi"("State(s) in Front (\"\")"="UI: Update Sampling Status\nData: Waveform Legends" ("State(s) in Front (\"\")"), "State(s) at Back (\"\")"=w1935) -> ("States Out"=w1934:string)  [unwired: 13 in]
            n918 = call <vilib>:"Add State(s) to Queue__jki_lib_state_machine.vi"("State(s) in Front (\"\")"=w1934, "State(s) in (\"\")"=w1940) -> ("States Out"=w1939:string)  [unwired: 13 in]
          }
          frame "Macro: Update Lockin Graphs" {
            n919 = Unbundle By Name(w1946) -> ("getAll.Results.Results (Dictionary)"=w1954:cluster{"key":string, "value":dbl[]}[])
            n920 = call "Dictionary to Plot Names.vi"("error in (no error)"=w1952, "Results (Dictionary)"=w1954) -> ("error out"=w1953:errorcluster, "Plot Names"=w1948:string[])  [unwired: 7 in, 1 out]
            n921 = call "Is Value Changed.vim"("value"=w1948) -> ("changed or first call?"=w1947:bool)
            n922 = Select(t="UI: Defer Panel Updates >> TRUE\nUI: Update Channel Ring\nUI: Update Lockin Graphs Legends\nUI: Update Lockin Graphs Colors\nUI: Defer Panel Updates >> FALSE" ("State(s) in Front (\"\")"), s=w1947, f="") -> (s? t:f=w1944:string)
            n923 = call <vilib>:"Add State(s) to Queue__jki_lib_state_machine.vi"("State(s) in Front (\"\")"="UI: Update Lockin Graphs" ("State(s) in Front (\"\")"), "State(s) at Back (\"\")"=w1944) -> ("States Out"=w1949:string)  [unwired: 13 in]
            n924 = call <vilib>:"Add State(s) to Queue__jki_lib_state_machine.vi"("State(s) in Front (\"\")"=w1949, "State(s) in (\"\")"=w1957) -> ("States Out"=w1956:string)  [unwired: 13 in]
          }
          frame "Macro: Save Configuration" {
            n925 = call <vilib>:"Add State(s) to Queue__jki_lib_state_machine.vi"("State(s) in Front (\"\")"="UI: Defer Panel Updates >> TRUE\nUI: Get Plot Visibility\nUI: UI to Cluster\nUI: UI to Cluster 2\nConfiguration: Write File\nUI: Defer Panel Updates >> FALSE", "State(s) in (\"\")"=w1963) -> ("States Out"=w1962:string)  [unwired: 13 in]
          }
          frame "Macro: Exit" {
            # "Exit Macro\n(This is called once, when the VI exits)"
            n926 = Unbundle By Name(w1966) -> ("Core.Close Panel on Exit?"=w1977:bool)
            n927 = Bundle By Name(cluster=w1966, "Core.Shutdown?"=TRUE) -> (w1967:T65)
            n928 = Select(t="UI: Front Panel State >> Open", s=w1977, f="") -> (s? t:f=w1964:string)
            n929 = call <vilib>:"Add State(s) to Queue__jki_lib_state_machine.vi"("State(s) in Front (\"\")"="Data: Cleanup\nEvents: Unregister\nProcess: Self Terminate", "State(s) in (\"\")"="Process: Sync", "State(s) at Back (\"\")"="Exit") -> ("States Out"=w1965:string)  [unwired: 12 in]
            n930 = call <vilib>:"Add State(s) to Queue__jki_lib_state_machine.vi"("State(s) in Front (\"\")"="Macro: Save Configuration", "State(s) in (\"\")"=w1964, "State(s) at Back (\"\")"=w1965) -> ("States Out"=w1974:string)  [unwired: 12 in]
            n931 = call <vilib>:"Add State(s) to Queue__jki_lib_state_machine.vi"("State(s) in Front (\"\")"=w1974, "State(s) in (\"\")"=w1980) -> ("States Out"=w1979:string)  [unwired: 13 in]
          }
          frame "---------- Process ----------" {
            # "Template Separator\n(You can make a copy of, or modify, this frame)"
            n932 = call <vilib>:"Add State(s) to Queue__jki_lib_state_machine.vi"("State(s) in (\"\")"=w1985) -> ("States Out"=w1984:string)  [unwired: 14 in]
          }
          frame "Process: Sync" {
            n933 = Unbundle By Name(w1993) -> ("SelfRef"=w1989:refnum<class "Instrument UI.Lockin.lvclass">)
            n934 = call <vilib>:"WaitOnProcessSync.vi"("error in (no error)"=w1988, "SMO"=w1989) -> ("error out"=w1987:errorcluster, "Don't run?"=w1992:bool)  [unwired: 7 in, 1 out]
            n935 = Select(t="Data: Cleanup\nEvents: Unregister\nExit", s=w1992, f="") -> (s? t:f=w1986:string)
            n936 = call <vilib>:"Add State(s) to Queue__jki_lib_state_machine.vi"("State(s) in Front (\"\")"=w1986, "State(s) in (\"\")"=w1996) -> ("States Out"=w1995:string)  [unwired: 13 in]
          }
          frame "Process: Self Terminate" {
            n937 = Unbundle By Name(w1998) -> ("SelfRef"=w1997:refnum<class "Instrument UI.Lockin.lvclass">)
            n938 = call <vilib>:"SelfTerminate.vi"("error in (no error)"=w2000, "SMO in"=w1997) -> ("error out"=w1999:errorcluster)  [unwired: 8 in, 1 out]
            n939 = call <vilib>:"Add State(s) to Queue__jki_lib_state_machine.vi"("State(s) in (\"\")"=w2003) -> ("States Out"=w2002:string)  [unwired: 14 in]
          }
          frame "---------- Events ----------" {
            # "Template Separator\n(You can make a copy of, or modify, this frame)"
            n940 = call <vilib>:"Add State(s) to Queue__jki_lib_state_machine.vi"("State(s) in (\"\")"=w2008) -> ("States Out"=w2007:string)  [unwired: 14 in]
          }
          frame "Events: Register" {
            # "Base Class Protected Events"
            n941 = Unbundle By Name(w2025) -> ("SelfRef"=w2021:refnum<class "Instrument UI.Lockin.lvclass">, "Lockin"=w2015:refnum<class "Instrument.Lockin.lvclass">)
            n942 = call <vilib>:"GetProtectedEvents.vi"("SMO"=w2021) -> ("error out"=w2022:errorcluster, "SMO Protected Events"=w2014:T69, "SMO out"=w2013:refnum<class "Instrument UI.Lockin.lvclass">)  [unwired: 8 in]
            n943 = call <userlib>:"Instrument.GetPublicEvents.vi"("Instrument"=w2015) -> ("error out"=w2020:errorcluster, "Instrument Public Events"=w2016:T70, "Instrument out"=w2017:refnum<class "Instrument.Lockin.lvclass">)  [unwired: 8 in]
            n944 = call <vilib>:"SMO.UI.GetPublicEvents.vi"("SMO.UI"=w2013) -> ("SMO.UI Public Events"=w2012:T71)  [unwired: 8 in, 2 out]
            n945 = call "Lockin.getDAQPublicEvents.vi"("Instrument.Lockin in"=w2017) -> ("error out"=w2010:errorcluster, "DAQ SMO Public Events"=w2011:T72, "DAQ Public Events"=w2009:T73)  [unwired: 7 in, 1 out]
            n946 = register-events(w2014, w2012, w2016, w2009, w2011) -> (reference out=w2024:refnum<event-registration>, error out=w2019:errorcluster)  [unwired: 2 in]
            n947 = Merge Errors(w2019, w2010, w2020, w2022, w2018) -> (w2023:errorcluster)
            n948 = call <vilib>:"Add State(s) to Queue__jki_lib_state_machine.vi"("State(s) in (\"\")"=w2027) -> ("States Out"=w2026:string)  [unwired: 14 in]
          }
          frame "Events: Unregister" {
            n949 = Unregister For Events(event registration refnum=w2030, error in=w2029) -> (error out=w2028:errorcluster)
            n950 = call <vilib>:"Add State(s) to Queue__jki_lib_state_machine.vi"("State(s) in (\"\")"=w2033) -> ("States Out"=w2032:string)  [unwired: 14 in]
          }
          frame "---------- Action ----------" {
            n951 = Unbundle By Name(w2034) -> ("SelfRef"=w2036:refnum<class "Instrument UI.Lockin.lvclass">)
            n952 = Bundle By Name(cluster=w2034, "SelfRef"=w2036) -> (w2035:T65)
            n953 = call <vilib>:"Add State(s) to Queue__jki_lib_state_machine.vi"("State(s) in (\"\")"=w2040) -> ("States Out"=w2039:string)  [unwired: 14 in]
          }
          frame "Action: ><><>Unhandled Controls<><><" {
            n954 = call <vilib>:"Add State(s) to Queue__jki_lib_state_machine.vi"("State(s) in (\"\")"=w2045) -> ("States Out"=w2044:string)  [unwired: 14 in]
          }
          frame "Action: Notify UI Closed" {
            # "Notify that the UI has been closed"
            n955 = Unbundle By Name(w2048) -> ("SelfRef"=w2049:refnum<class "Instrument UI.Lockin.lvclass">)
            n956 = call <vilib>:"Hide.vi"("error in (no error)"=w2047, "SMO.UI"=w2049) -> ("error out"=w2046:errorcluster)  [unwired: 8 in, 1 out]
            n957 = call <vilib>:"Add State(s) to Queue__jki_lib_state_machine.vi"("State(s) in (\"\")"=w2052) -> ("States Out"=w2051:string)  [unwired: 14 in]
          }
          frame "Action: Command" {
            n958 = Unbundle By Name(w2060) -> ("Lockin"=w2058:refnum<class "Instrument.Lockin.lvclass">, "Message.Command"=w2057:variant, "Message.Data"=w2056:variant)
            n959 = call "Lockin.Local Client.vim"("error in (no error)"=w2055, "Data"=w2056, "Command"=w2057, "Instrument.Lockin in"=w2058) -> ("error out"=w2054:errorcluster, "Instrument.Lockin out"=w2053:refnum<class "Instrument.Lockin.lvclass">)  [unwired: 6 in]
            n960 = Bundle By Name(cluster=w2060, "Lockin"=w2053) -> (w2061:T65)
            n961 = call <vilib>:"Add State(s) to Queue__jki_lib_state_machine.vi"("State(s) in Front (\"\")"="" ("State(s) in Front (\"\")"), "State(s) in (\"\")"=w2064) -> ("States Out"=w2063:string)  [unwired: 13 in]
          }
          frame "Action: IDN" {
            n962 = Unbundle By Name(w2072) -> ("Lockin"=w2070:refnum<class "Instrument.Lockin.lvclass">)
            n963 = call <userlib>:"IDN.vi"("error in (no error)"=w2069, "Instrument in"=w2070) -> ("error out"=w2068:errorcluster, "IDN"=w2066:T74, "Instrument in"=w2067:refnum<class "Instrument.Lockin.lvclass">)  [unwired: 7 in]
            n964 = Unbundle By Name(w2066) -> ("serial"=→"System Serial Number":string)
            n965 = Bundle By Name(cluster=w2072, "Lockin"=w2067) -> (w2073:T65)
            n966 = call <vilib>:"Add State(s) to Queue__jki_lib_state_machine.vi"("State(s) in Front (\"\")"="" ("State(s) in Front (\"\")"), "State(s) in (\"\")"=w2076) -> ("States Out"=w2075:string)  [unwired: 13 in]
          }
          frame "Action: State" {
            n967 = Scan From String(input string=w2081, default 1=State--enum."start" ("State")) -> (output 1=w2078:T29)  [unwired: 3 in, 3 out]
            n968 = Bundle By Name(cluster=T37 {"State"=enum."start"} ("setState"), "State"=w2078) -> (w2077:T37)
            n969 = Bundle By Name(cluster=w2083, "Message.Command"=Lockin.Commands--Enum."setState" ("Locking.Commands"), "Message.Data"=w2077) -> (w2084:T65)
            n970 = call <vilib>:"Add State(s) to Queue__jki_lib_state_machine.vi"("State(s) in (\"\")"=w2088) -> ("States Out"=w2087:string)  [unwired: 14 in]
          }
          frame "Action: show DAQ UI" {
            n971 = Scan From String(input string=w2092, default 1=T40 FALSE ("showDAQUI")) -> (output 1=w2089:T40)  [unwired: 3 in, 3 out]
            n972 = Bundle By Name(cluster=w2093, "Message.Command"=Lockin.Commands.Local--Enum."showUI" ("Locking.Commands.Local"), "Message.Data"=w2089) -> (w2094:T65)
            n973 = call <vilib>:"Add State(s) to Queue__jki_lib_state_machine.vi"("State(s) in (\"\")"=w2098) -> ("States Out"=w2097:string)  [unwired: 14 in]
          }
          frame "Action: Logging" {
            n974 = Scan From String(input string=w2110, default 1=FALSE ("showDAQUI")) -> (output 1=w2103:bool)  [unwired: 3 in, 3 out]
            n975 = Select(t=Lockin.Commands--Enum."startLogging" ("Locking.Commands"), s=w2103, f=Lockin.Commands--Enum."stopLogging" ("Locking.Commands")) -> (s? t:f=w2104:T38)
            n976 = Bundle By Name(cluster=T41 {"interval"=1} ("setLogging"), "interval"=u32 1000 ("LogMode")) -> (w2107:T41)
            n977 = To Variant(anything=w2107) -> (Variant=w2101:variant)
            n978 = Select(t=w2101, s=w2103, f=variant) -> (s? t:f=w2100:variant)
            n979 = Bundle By Name(cluster=w2111, "Message.Command"=w2104, "Message.Data"=w2100) -> (w2112:T65)
            n980 = call <vilib>:"Add State(s) to Queue__jki_lib_state_machine.vi"("State(s) in (\"\")"=w2116) -> ("States Out"=w2115:string)  [unwired: 14 in]
          }
          frame "Action: Log Configuration" {
            n981 = Bundle By Name(cluster=w2119, "Message.Command"=Lockin.Commands--Enum."logConfiguration" ("Locking.Commands"), "Message.Data"=variant) -> (w2120:T65)
            n982 = call <vilib>:"Add State(s) to Queue__jki_lib_state_machine.vi"("State(s) in (\"\")"=w2124) -> ("States Out"=w2123:string)  [unwired: 14 in]
          }
          frame "Action: Auto DAQ" {
            n983 = Bundle By Name(cluster=w2126, "Message.Command"=Lockin.Commands.Local--Enum."autoConfigureDAQ" ("Locking.Commands.Local")) -> (w2127:T65)
            n984 = call <vilib>:"Add State(s) to Queue__jki_lib_state_machine.vi"("State(s) in (\"\")"=w2131) -> ("States Out"=w2130:string)  [unwired: 14 in]
          }
          frame "Action: DAQ Config" {
            n985 = Unbundle By Name(w2134) -> ("UI Config.DAQ.Configuration"=w2132:T9)
            n986 = Bundle By Name(cluster=w2134, "Message.Command"=Lockin.Commands--Enum."setDAQ" ("Locking.Commands"), "Message.Data"=w2132) -> (w2135:T65)
            n987 = call <vilib>:"Add State(s) to Queue__jki_lib_state_machine.vi"("State(s) in (\"\")"=w2139) -> ("States Out"=w2138:string)  [unwired: 14 in]
          }
          frame "Action: AI Channels" {
            n988 = Unbundle By Name(w2142) -> ("UI Config.Channels.Cfg_AI"=w2141:T4)
            n989 = Bundle By Name(cluster=w2142, "Message.Command"=Lockin.Commands.Local--Enum."setAI" ("Locking.Commands.Local"), "Message.Data"=w2141) -> (w2143:T65)
            n990 = call <vilib>:"Add State(s) to Queue__jki_lib_state_machine.vi"("State(s) in (\"\")"=w2147) -> ("States Out"=w2146:string)  [unwired: 14 in]
          }
          frame "Action: AO Channels" {
            n991 = Unbundle By Name(w2150) -> ("UI Config.Channels.Cfg_AO"=w2148:T6)
            n992 = Bundle By Name(cluster=w2150, "Message.Command"=Lockin.Commands--Enum."setAO" ("Locking.Commands"), "Message.Data"=w2148) -> (w2151:T65)
            n993 = call <vilib>:"Add State(s) to Queue__jki_lib_state_machine.vi"("State(s) in (\"\")"=w2155) -> ("States Out"=w2154:string)  [unwired: 14 in]
          }
          frame "Action: AO Zero Amplitude" {
            n994 = Unbundle By Name(w2156) -> ("UI Config.Channels.Cfg_AO"=w2159:T6)
            n995 = for {
              tunnel: w2159 -> [w2168] mode=indexing
              tunnel: [w2166] -> w2158 mode=indexing
              n996 = Bundle By Name(cluster=w2168, "Amplitude"=0.0 ("element")) -> (w2166:T7)
            }
            n997 = Bundle By Name(cluster=w2156, "Message.Command"=Lockin.Commands--Enum."setAO" ("Enum"), "Message.Data"=w2158) -> (w2157:T65)
            n998 = call <vilib>:"Add State(s) to Queue__jki_lib_state_machine.vi"("State(s) in Front (\"\")"="", "State(s) in (\"\")"=w2165) -> ("States Out"=w2164:string)  [unwired: 13 in]
          }
          frame "Action: REF Channels" {
            n999 = Unbundle By Name(w2173) -> ("UI Config.Channels.Cfg_REF"=w2171:T2, "UI Config.DAQ.cfg.Sampling.Sampling"=w2169:T49)
            n1000 = call "Calculate Output Sampling.vi"("sampling info"=w2169, "Cfg_REF"=w2171) -> ("Cfg_REF out"=w2170:T2)  [unwired: 8 in, 1 out]
            n1001 = Bundle By Name(cluster=w2173, "Message.Command"=Lockin.Commands--Enum."setREF" ("Locking.Commands"), "Message.Data"=w2170) -> (w2174:T65)
            n1002 = call <vilib>:"Add State(s) to Queue__jki_lib_state_machine.vi"("State(s) in (\"\")"=w2178) -> ("States Out"=w2177:string)  [unwired: 14 in]
          }
          frame "Action: Sweep" {
            n1003 = Unbundle By Name(w2181) -> ("UI Config.Sweep"=w2179:T55)
            n1004 = Bundle By Name(cluster=w2181, "Message.Command"=Lockin.Commands--Enum."setSweep" ("Locking.Commands"), "Message.Data"=w2179) -> (w2182:T65)
            n1005 = call <vilib>:"Add State(s) to Queue__jki_lib_state_machine.vi"("State(s) in (\"\")"=w2186) -> ("States Out"=w2185:string)  [unwired: 14 in]
          }
          frame "Action: Sampling" {
            w2191 = Lockin.Commands--Enum."setSampling"  # Lockin.Commands
            n1006 = Unbundle By Name(w2192) -> ("UI Config.DAQ.cfg.Sampling.Sampling"=w2188:T49)
            n1007 = Bundle By Name(cluster=w2188, "Fs"="Fs (S/s) (buffer)", "#s"="#s (S) (buffer)") -> (w2187:T49)
            n1008 = Bundle By Name(cluster=w2192, "Message.Command"=w2191, "Message.Data"=w2187) -> (w2193:T65)
            n1009 = call <vilib>:"Add State(s) to Queue__jki_lib_state_machine.vi"("State(s) in (\"\")"=w2197) -> ("States Out"=w2196:string)  [unwired: 14 in]
          }
          frame "Action: Sampling Mode" {
            n1010 = Unbundle By Name(w2202) -> ("UI Config.DAQ.cfg.Sampling.sample mode"=w2199:i32)
            n1011 = Bundle By Name(cluster=T42 {"SampleMode"=10123} ("setSampleMode"), "SampleMode"=w2199) -> (w2198:T42)
            n1012 = Bundle By Name(cluster=w2202, "Message.Command"=Lockin.Commands.Local--Enum."setSamplingMode" ("Enum"), "Message.Data"=w2198) -> (w2203:T65)
            n1013 = call <vilib>:"Add State(s) to Queue__jki_lib_state_machine.vi"("State(s) in (\"\")"=w2207) -> ("States Out"=w2206:string)  [unwired: 14 in]
          }
          frame "Action: Sampling Fs Mode" {
            n1014 = Unbundle By Name(w2212) -> ("UI Config.DAQ.cfg.Sampling.Fs Mode"=w2209:T15)
            n1015 = Bundle By Name(cluster=T44 {"FsMode"=enum."Manual"} ("setSampleFsMode"), "FsMode"=w2209) -> (w2208:T44)
            n1016 = Bundle By Name(cluster=w2212, "Message.Command"=Lockin.Commands--Enum."setSamplingFsMode" ("Commands"), "Message.Data"=w2208) -> (w2213:T65)
            n1017 = call <vilib>:"Add State(s) to Queue__jki_lib_state_machine.vi"("State(s) in (\"\")"=w2217) -> ("States Out"=w2216:string)  [unwired: 14 in]
          }
          frame "Action: Sampling Fs Multiplier" {
            n1018 = Unbundle By Name(w2220) -> ("UI Config.DAQ.cfg.Sampling.Fs Multiplier"=w2219:dbl)
            n1019 = Bundle By Name(cluster=w2220, "Message.Command"=Lockin.Commands.Local--Enum."setSamplingFsMultiplier" ("Locking.Commands.Local"), "Message.Data"=w2219) -> (w2221:T65)
            n1020 = call <vilib>:"Add State(s) to Queue__jki_lib_state_machine.vi"("State(s) in (\"\")"=w2225) -> ("States Out"=w2224:string)  [unwired: 14 in]
          }
          frame "Action: Sampling Fs Output" {
            n1021 = Unbundle By Name(w2234) -> ("UI Config.Channels.Cfg_REF"=w2232:T2, "UI Config.DAQ.cfg.Sampling.Sampling"=w2231:T49)
            n1022 = call "Calculate Output Sampling.vi"("sampling info"=w2231, "Cfg_REF"=w2232) -> ("Filter Parameters"=w2230:T75)  [unwired: 8 in, 1 out]
            n1023 = Unbundle By Name(w2230) -> ("Fs.Output (S/s)"=w2226:dbl, "Settling Time (s)"=→"Settling Time (s)":dbl, "Noise Bandwidth (Hz)"=→"Noise BW (Hz)":dbl, "-3dB Bandwidth (Hz)"=→"-3dB BW (Hz)":dbl)
            "Fs Output (S/s)" <- w2226
            n1024 = Bundle By Name(cluster=w2234, "Message.Command"=Lockin.Commands.Local--Enum."setSamplingFsOutput" ("Locking.Commands.Local"), "Message.Data"=w2226, "UI Config.DAQ.cfg.Sampling.Fs.Output"=w2226) -> (w2235:T65)
            n1025 = call <vilib>:"Add State(s) to Queue__jki_lib_state_machine.vi"("State(s) in (\"\")"=w2239) -> ("States Out"=w2238:string)  [unwired: 14 in]
          }
          frame "Action: Sampling Refresh Rate" {
            n1026 = Unbundle By Name(w2242) -> ("UI Config.DAQ.cfg.Sampling.Refresh Rate (Hz)"=w2241:dbl)
            n1027 = Bundle By Name(cluster=w2242, "Message.Command"=Lockin.Commands.Local--Enum."setSamplingRefreshRate" ("Locking.Commands.Local"), "Message.Data"=w2241) -> (w2243:T65)
            n1028 = call <vilib>:"Add State(s) to Queue__jki_lib_state_machine.vi"("State(s) in (\"\")"=w2247) -> ("States Out"=w2246:string)  [unwired: 14 in]
          }
          frame "Action: Sampling Decimation Pre DSP" {
            n1029 = Unbundle By Name(w2250) -> ("UI Config.DAQ.cfg.Sampling.Decimation.PreDSP"=w2249:i32)
            n1030 = Bundle By Name(cluster=w2250, "Message.Command"=Lockin.Commands.Local--Enum."setSamplingDecimationPreDSP" ("Locking.Commands.Local"), "Message.Data"=w2249) -> (w2251:T65)
            n1031 = call <vilib>:"Add State(s) to Queue__jki_lib_state_machine.vi"("State(s) in (\"\")"=w2255) -> ("States Out"=w2254:string)  [unwired: 14 in]
          }
          frame "Action: Sampling Decimation Post DSP" {
            n1032 = Unbundle By Name(w2258) -> ("UI Config.DAQ.cfg.Sampling.Decimation.PostDSP"=w2257:i32)
            n1033 = Bundle By Name(cluster=w2258, "Message.Command"=Lockin.Commands.Local--Enum."setSamplingDecimationPostDSP" ("Locking.Commands.Local"), "Message.Data"=w2257) -> (w2259:T65)
            n1034 = call <vilib>:"Add State(s) to Queue__jki_lib_state_machine.vi"("State(s) in (\"\")"=w2263) -> ("States Out"=w2262:string)  [unwired: 14 in]
          }
          frame "Action: AI Simulate Mode" {
            n1035 = Unbundle By Name(w2266) -> ("UI Config.DAQ.Simulation mode"=w2265:T16)
            n1036 = Bundle By Name(cluster=w2266, "Message.Command"=Lockin.Commands.Local--Enum."setSimulationMode" ("Locking.Commands.Local"), "Message.Data"=w2265) -> (w2267:T65)
            n1037 = call <vilib>:"Add State(s) to Queue__jki_lib_state_machine.vi"("State(s) in (\"\")"=w2271) -> ("States Out"=w2270:string)  [unwired: 14 in]
          }
          frame "Action: Limit Amplitude" {
            n1038 = Unbundle By Name(w2274) -> ("UI Config.Limit Amplitude"=w2273:T52)
            n1039 = Bundle By Name(cluster=w2274, "Message.Command"=Lockin.Commands.Local--Enum."setAmplitudeLimit" ("Locking.Commands.Local"), "Message.Data"=w2273) -> (w2275:T65)
            n1040 = call <vilib>:"Add State(s) to Queue__jki_lib_state_machine.vi"("State(s) in (\"\")"=w2279) -> ("States Out"=w2278:string)  [unwired: 14 in]
          }
          frame "Action: Limit DC" {
            n1041 = Unbundle By Name(w2282) -> ("UI Config.Limit DC"=w2281:T53)
            n1042 = Bundle By Name(cluster=w2282, "Message.Command"=Lockin.Commands.Local--Enum."setDCLimit" ("Locking.Commands.Local"), "Message.Data"=w2281) -> (w2283:T65)
            n1043 = call <vilib>:"Add State(s) to Queue__jki_lib_state_machine.vi"("State(s) in (\"\")"=w2287) -> ("States Out"=w2286:string)  [unwired: 14 in]
          }
          frame "Action: Link Frequencies" {
            n1044 = Unbundle By Name(w2290) -> ("UI Config.Link Frequencies"=w2289:T54)
            n1045 = Bundle By Name(cluster=w2290, "Message.Command"=Lockin.Commands.Local--Enum."setFrequencyLink" ("Locking.Commands.Local"), "Message.Data"=w2289) -> (w2291:T65)
            n1046 = call <vilib>:"Add State(s) to Queue__jki_lib_state_machine.vi"("State(s) in (\"\")"=w2295) -> ("States Out"=w2294:string)  [unwired: 14 in]
          }
          frame "Action: Duty Cycle" {
            n1047 = Unbundle By Name(w2298) -> ("UI Config.Function Option"=w2297:T56)
            n1048 = Bundle By Name(cluster=w2298, "Message.Command"=Lockin.Commands.Local--Enum."setDutyCycle" ("Locking.Commands.Local"), "Message.Data"=w2297) -> (w2299:T65)
            n1049 = call <vilib>:"Add State(s) to Queue__jki_lib_state_machine.vi"("State(s) in (\"\")"=w2303) -> ("States Out"=w2302:string)  [unwired: 14 in]
          }
          frame "Action: PreFilter" {
            n1050 = Unbundle By Name(w2306) -> ("UI Config.PreFilter"=w2305:T50)
            n1051 = Bundle By Name(cluster=w2306, "Message.Command"=Lockin.Commands.Local--Enum."setPreFilter" ("Locking.Commands.Local"), "Message.Data"=w2305) -> (w2307:T65)
            n1052 = call <vilib>:"Add State(s) to Queue__jki_lib_state_machine.vi"("State(s) in (\"\")"=w2311) -> ("States Out"=w2310:string)  [unwired: 14 in]
          }
          frame "Action: Input Gain" {
            n1053 = Unbundle By Name(w2315) -> ("UI Config.Amplifers.Gain_AI"=w2313:T17)
            n1054 = for {
              tunnel: w2313 -> [w2322] mode=indexing
              tunnel: [w2321] -> w2312 mode=indexing
              n1055 = Unbundle By Name(w2322) -> ("Gain"=w2321:dbl)
            }
            n1056 = Bundle By Name(cluster=w2315, "Message.Command"=Lockin.Commands--Enum."setInputGain" ("Locking.Commands"), "Message.Data"=w2312) -> (w2316:T65)
            n1057 = call <vilib>:"Add State(s) to Queue__jki_lib_state_machine.vi"("State(s) in (\"\")"=w2320) -> ("States Out"=w2319:string)  [unwired: 14 in]
          }
          frame "Action: Output Gain" {
            n1058 = Unbundle By Name(w2326) -> ("UI Config.Amplifers.Gain_AO"=w2324:T17)
            n1059 = for {
              tunnel: w2324 -> [w2333] mode=indexing
              tunnel: [w2332] -> w2323 mode=indexing
              n1060 = Unbundle By Name(w2333) -> ("Gain"=w2332:dbl)
            }
            n1061 = Bundle By Name(cluster=w2326, "Message.Command"=Lockin.Commands--Enum."setOutputGain" ("Locking.Commands"), "Message.Data"=w2323) -> (w2327:T65)
            n1062 = call <vilib>:"Add State(s) to Queue__jki_lib_state_machine.vi"("State(s) in (\"\")"=w2331) -> ("States Out"=w2330:string)  [unwired: 14 in]
          }
          frame "Action: Offset" {
            n1063 = Unbundle By Name(w2335) -> ("UI Config.Amplifers.Offset_AI"=w2336:T17)
            n1064 = for {
              tunnel: w2336 -> [w2344] mode=indexing
              tunnel: [w2343] -> w2334 mode=indexing
              n1065 = Unbundle By Name(w2344) -> ("Gain"=w2343:dbl)
            }
            n1066 = Bundle By Name(cluster=w2335, "Message.Command"=Lockin.Commands.Local--Enum."setOffset" ("Locking.Commands.Local"), "Message.Data"=w2334) -> (w2338:T65)
            n1067 = call <vilib>:"Add State(s) to Queue__jki_lib_state_machine.vi"("State(s) in (\"\")"=w2342) -> ("States Out"=w2341:string)  [unwired: 14 in]
          }
          frame "Action: Offset Mode" {
            n1068 = Scan From String(input string=w2348, default 1=Offset_Mode--Enum."Measure" ("Offset Mode")) -> (output 1=w2347:T31)  [unwired: 3 in, 3 out]
            n1069 = Build Array(w2347) -> (w2346:T31[])
            n1070 = Bundle By Name(cluster=w2350, "Message.Command"=Lockin.Commands.Local--Enum."setOffsetMode" ("Locking.Commands.Local"), "Message.Data"=w2346) -> (w2351:T65)
            n1071 = call <vilib>:"Add State(s) to Queue__jki_lib_state_machine.vi"("State(s) in (\"\")"=w2355) -> ("States Out"=w2354:string)  [unwired: 14 in]
          }
          frame "Action: Calibrate" {
            n1072 = Scan From String(input string=w2358, default 1=PrivateEvents--DAQ.setCalibration."Check" ("setCalibration")) -> (output 1=w2357:T32)  [unwired: 3 in, 3 out]
            n1073 = Bundle By Name(cluster=w2360, "Message.Command"=Lockin.Commands.Local--Enum."setCalibration" ("Locking.Commands.Local"), "Message.Data"=w2357) -> (w2361:T65)
            n1074 = call <vilib>:"Add State(s) to Queue__jki_lib_state_machine.vi"("State(s) in (\"\")"=w2365) -> ("States Out"=w2364:string)  [unwired: 14 in]
          }
          frame "Action: Zero Phase" {
            n1075 = Bundle By Name(cluster=w2367, "Message.Command"=Lockin.Commands.Local--Enum."zeroPhase" ("Locking.Commands.Local")) -> (w2368:T65)
            n1076 = call <vilib>:"Add State(s) to Queue__jki_lib_state_machine.vi"("State(s) in (\"\")"=w2372) -> ("States Out"=w2371:string)  [unwired: 14 in]
          }
          frame "Action: Power Spectrum" {
            n1077 = Unbundle By Name(w2396) -> ("getAll.Waveforms.AO"=w2385:waveform(dbl)[], "getAll.Waveforms.AI"=w2381:waveform(dbl)[], "Waveform Charts"=w2378:waveform(dbl)[][])
            n1078 = call "Is Value Changed.vim"("value"="PS Display") -> ("changed or first call?"=w2384:bool)
            n1079 = case shown="\"AI\"" "PS Display" {
              tunnel: w2385 -> [w2409 _ _ _ _ _]
              tunnel: [w2409 w2410 w2411 w2415 w2418 w2421] -> w2382
              tunnel: w2381 -> [_ w2410 _ _ _ _]
              tunnel: w2378 -> [_ _ w2412 w2416 w2419 w2422]
              frame "AO", Default {
              }
              frame "AI" {
              }
              frame "X" {
                n1080 = Index Array(array=w2412, index (row)=0) -> (element=w2411:waveform(dbl)[])  [unwired: 1 in]
              }
              frame "Y" {
                n1081 = Index Array(array=w2416, index (row)=1) -> (element=w2415:waveform(dbl)[])  [unwired: 1 in]
              }
              frame "R" {
                n1082 = Index Array(array=w2419, index (row)=2) -> (element=w2418:waveform(dbl)[])  [unwired: 1 in]
              }
              frame "Theta" {
                n1083 = Index Array(array=w2422, index (row)=3) -> (element=w2421:waveform(dbl)[])  [unwired: 1 in]
              }
            }
            n1084 = Bundle By Name(cluster=T45 {"averaging mode"=enum."No averaging", "weighting mode"=enum."Exponential", "number of averages"=10} ("averaging parameters"), "averaging mode"="averaging mode", "weighting mode"="weighting mode", "number of averages"="# averages") -> (w2389:T45)
            n1085 = Or(x="restart", y=w2384) -> (x .or. y?=w2373:bool)
            n1086 = call-poly <vilib>:"FFT Power Spectrum and PSD.vi"("export mode"="export mode", "averaging parameters"=w2389, "restart averaging (F)"=w2373, "error in (no error)"=w2395, "dB On (F)"=TRUE, "window"="window", "time signals"=w2382) -> ("error out"=w2376:errorcluster, "averages completed"=→"averages":dbl, "averaging done"=→"done?":bool, "Power Spectrum / PSD"=w2377:cluster{"f0":dbl, "df":dbl, "magnitude":dbl[]}[])  [unwired: 1 in]
            "PS Waveform" <- w2377
            n1087 = case shown="True" w2373 {
              frame False {
              }
              frame True {
                w2400 = u8 1 ("X Scale.Scale Fit")
                n1088 = property on="PS Waveform" class="WFGraph (strict)"("XScale.ScaleFit"=w2400, "YScale.ScaleFit"=w2400) -> ()  [unwired: 2 in, 2 out]
              }
            }
            n1089 = case shown="True" "chart?" {
              tunnel: w2377 -> [_ w2408]
              tunnel: w2376 -> [w2402 w2407]
              tunnel: [w2402 w2406] -> w2375
              frame False {
                n1090 = local write "PS Chart"(dbl[][] [] ("Waveform Chart")) -> ()
              }
              frame True {
                n1091 = control-ref of="PS Waveform"() -> (w2405:refnum<vi>)
                n1092 = call "PS Chart.vi"("all?"="chart all?", "error in (no error)"=w2407, "Power Spectrum / PSD"=w2408, "WFGraph (WDT) in"=w2405) -> ("error out"=w2406:errorcluster, "Chart"=→"PS Chart":dbl[][])  [unwired: 6 in]
              }
            }
            n1093 = call <vilib>:"Add State(s) to Queue__jki_lib_state_machine.vi"("State(s) in (\"\")"=w2399) -> ("States Out"=w2398:string)  [unwired: 14 in]
          }
          frame "Action: Route" {
            n1094 = Unbundle By Name(w2423) -> ("SelfRef"=w2425:refnum<class "Instrument UI.Lockin.lvclass">)
            n1095 = Bundle By Name(cluster=w2423, "SelfRef"=w2425) -> (w2424:T65)
            n1096 = call <vilib>:"Add State(s) to Queue__jki_lib_state_machine.vi"("State(s) in (\"\")"=w2429) -> ("States Out"=w2428:string)  [unwired: 14 in]
          }
          frame "Action: PLL" {
            n1097 = Unbundle By Name(w2430) -> ("SelfRef"=w2432:refnum<class "Instrument UI.Lockin.lvclass">)
            n1098 = Bundle By Name(cluster=w2430, "SelfRef"=w2432) -> (w2431:T65)
            n1099 = call <vilib>:"Add State(s) to Queue__jki_lib_state_machine.vi"("State(s) in (\"\")"=w2436) -> ("States Out"=w2435:string)  [unwired: 14 in]
          }
        }
      }
    }
    frame Error {
    }
  }
  n1100 = call-parent "Process.vi"("error in"=w5, "Instrument UI in"=w4) -> ("error out"=w2:errorcluster, "Instrument UI out"=→"Lockin.UI out":refnum<class "Instrument UI.Lockin.lvclass">)  [unwired: 8 in]
  n1101 = Merge Errors(w2, w1) -> (→"error out":errorcluster)
